vi "Beampointing_sam_edit.vi"() -> ()   [LabVIEW 2020]
uses:
  Ctrs/beam detection.ctl
  GUI_Beampointing_single_TRA/Ctrs/move.ctl
  Shared/GUI_Template/GUI_master/tcp_new_data_event.ctl
  Shared/GUI_Template/GUI_master/tcp new data cluster.ctl
  Ctrs/thresholds.ctl
  Ctrs/Detection all.ctl
  Ctrs/BP configuration.ctl
  General GUIs/Device GUIs/GUI_Cameras/Controls/Crosshair type def.ctl
  <userlib>/_OpenG.lib/array/array.llb/Filter 1D Array with Scalar (String)__ogtk.vi
  <userlib>/_OpenG.lib/array/array.llb/Sort 1D Array (DBL)__ogtk.vi
  <userlib>/_OpenG.lib/array/array.llb/Reorder 1D Array2 (Variant)__ogtk.vi
  <userlib>/_OpenG.lib/file/file.llb/File Exists - Scalar__ogtk.vi
  <userlib>/_OpenG.lib/array/array.llb/Remove Duplicates from 1D Array (String)__ogtk.vi
  <userlib>/_OpenG.lib/file/file.llb/Strip Path Extension - String__ogtk.vi
  <vilib>/Analysis/NI_AALBase.lvlib
  <vilib>/vision/NI_Vision_Development_Module.lvlib
  <vilib>/Utility/file.llb/Write To Spreadsheet File (string).vi
panel:
  in  "pixel calib":dbl
  out "A2y":dbl
  out "A1y":dbl
  out "A2x":dbl
  out "A1x":dbl
  in  "y'":dbl
  in  "x'":dbl
  in  "y":dbl
  in  "x":dbl
  in  "distance to target plane":dbl
  in  "seperation":dbl
  in  "downstream mirror":dbl
  in  "upstream mirror":dbl
  in  "Load Config 2":bool
  out "error out":errorcluster
  in  "active CCDs":i32(listbox)
  out "Prev State":string
  out "tcp data event 2":T1
  out "error out 3":errorcluster
  out "cam means":sgl[](array[numeric])
  in  "save path":path=path "W:/BP_DATA"
  out "millisecond timer value":u32
  out "motor refs 3":refnum<vi>[](array[refnum])
  in  "active man refs":cluster{"Ref X":refnum<vi>, "Ref Y":refnum<vi>}
  in  "#imgs avd so far":dbl
  out "Current State":string
  out "CCDs":string[](array[string])
  in  "GUIdevice 12":string
  in  "GUIdevice 11":string
  in  "GUIdevice 10":string
  in  "GUIdevice 9":string
  out "error out 2":errorcluster
  out "Names":string[](array[string])
  out "Box":T2(array[cluster])
  in  "Tab Cams":T3(tab)=enum."Main"
  in  "Cameras and motors":T4(array[cluster]) {"Motor Alias Y" items=["SHG-angle", "compensation-plate-x", "compensation-plate-y", "Stage [um]", "grating angle", "AttenuatorWavelplate", "Delay", "micrometer", "rail position", "Amp3 North", "djjdjd", "drive grating 2 trans", "speed_translation", "speed_rot_grating2", "speed_rot_grating1", "drive grating 2 rot", "drive grating 1 rot", "jet x", "jet y", "jet z", "ESP2_1_blade", "ESP2_2_target rotation", "home1", "ESP2_3_Scatter ST4 Move", "ESP3_3_mode z position", "com", "ESP3_1_Scatter_Mirror_Z", "ESP3_2", "ESP6_1_scatter ST4 x/hor", "ESP6_2_scatter ST4 y/vert", "ESP6_3_scatter mode z", "VISA", "S1C1 x", "S1C1 y", "S1C1 z", "S1C2 x", "S1C2 y", "S1C2 z", "S1C3 x", "S1C3 y", "S1C3 z", "S1C4 x", "S1C4 y", "S1C4 z", "S2C1 x", "S2C1 y", "S2C1 z", "S2C2 x", "S2C2 y", "S2C2 z", "S2C3 x", "S2C3 y", "S2C3 z", "S2C4 x", "S2C4 y", "S2C4 z", "S3C1 x", "S3C1 y", "S3C1 z", "S3C2 x", "S3C2 y", "S3C2 z", "S3C3 x", "S3C3 y", "S3C3 z", "S3C4 x", "S3C4 y", "S3C4 z", "S4C1 x", "S4C1y", "S4C1 z", "S4C2 x", "S4C2 y", "S4C2 z", "S4C3 x", "S4C3 y", "S4C3 z", "S4C4 x", "S4C4 y", "S4C4 z", "S5C1 x", "S5C1 y", "S5C1 z", "S5C2 x", "S5C2 y", "S5C2 z", "S5C3 x", "S5C3 y", "S5C3 z", "S5C4 x", "S5C4 y", "S5C4 z", "S1C1", "S1C2", "S1C3", "S1C4", "S2C1", "S2C2", "S2C3", "S2C4", "S3C1", "S3C2", "S3C3", "S3C4", "S4C1", "S4C2", "S4C3", "S4C4", "S5C1", "S5C2", "S5C3", "S5C4", "Stepsize 1", "Stepsize 2", "Stepsize 3", "VISA", "S1C1", "S1C2", "S1C3", "S1C4", "S2C1", "S2C2", "S2C3", "S2C4", "S3C1", "S3C2", "S3C3", "S3C4", "S4C1", "S4C2", "S4C3", "S4C4", "S5C1", "S5C2", "S5C3", "S5C4", "kHz EC wedge", "Fiber Mode", "XH2", "ND6", "XH4", "d-scan wedge", "EC wedge", "Lanex", "Gentec", "ModeImager", "Magnet", "ProbeDelay", "x position", "y position", "not working", "LaserDiodeX", "LaserDiodeY", "DelayStage (mm)", "Focus_Beam_2 (mm)", "Hex_x", "Hex_y", "Hex_z", "Hex_u", "Hex_v", "Hex_w", "Mode_Image_pos (mm)", "Jet X", "Jet Y", "Jet Z", "Amp2_out_Y", "Amp3_in_X", "Amp2_out_X", "Amp3_in_Y", "Amp4_in_X", "Amp4_in_Y", "Amp4_in_X", "Gaia2_South_Y", "Gaia3_South_X", "Gaia3_South_Y", "Gaia4_South_X", "Gaia4_South_Y", "Amp2_in_X", "Not Working", "Gaia3_North_X", "Gaia3_North_Y", "Gaia4_North_X", "Gaia4_North_Y", "Expanderin_1_X", "Expanderin_1_Y", "weak current", "Amp4_Out_Y", "Gaia2_North_X", "Gaia2_North_Y", "Amp4_out_X", "Amp2_in_Y", "Gaia2_South_X", "Stretcher_Out_X", "Not_Working", "Stretcher_Out_Y", "JetBladeHeight", "Probe far X", "Probe far Y", "Probe near X", "Probe near Y", "Seed in X", "Seed in Y", "Probe delay X", "Probe delay Y", "Seed Lens Z", "SeedWaveplateRot", "Broken", "SeedPrismBroken", "SeedPrismY", "SeedPrismX", "BCaveDiodeM2Horizontal", "BCaveDiodeM2Vertical", "BCaveDiodeM1Vertical", "BCaveDiodeM1Horizontal", "Grating separation (um)", "Grating1 angle", "Grating2 angle", "Jet_X (mm)", "Jet_Y (mm)", "Jet_Z (mm)", "Prepulse stage", "LegendCompressor (mm)", "devport", "ModeImager", "JetBlade", "ProbeDelay", "1", "TubeIn-x", "TubeIn-y", "CompIn-x", "CompIn-y", "stepSize", "Beamline_In-x", "Beamline_In-y", "Beamline_Out-y", "Beamline_Out-x", "OAPin2-x", "OAPin2-y", "Chassi IP", "BCaveIn-X", "BCaveIn-Y", "OAPIn1-X", "OAPIn1-Y", "DMSurface-X", "DMSurface-Y", "testzaber"]; "Motor Alias X" items=["SHG-angle", "compensation-plate-x", "compensation-plate-y", "Stage [um]", "grating angle", "AttenuatorWavelplate", "Delay", "micrometer", "rail position", "Amp3 North", "djjdjd", "drive grating 2 trans", "speed_translation", "speed_rot_grating2", "speed_rot_grating1", "drive grating 2 rot", "drive grating 1 rot", "jet x", "jet y", "jet z", "ESP2_1_blade", "ESP2_2_target rotation", "home1", "ESP2_3_Scatter ST4 Move", "ESP3_3_mode z position", "com", "ESP3_1_Scatter_Mirror_Z", "ESP3_2", "ESP6_1_scatter ST4 x/hor", "ESP6_2_scatter ST4 y/vert", "ESP6_3_scatter mode z", "VISA", "S1C1 x", "S1C1 y", "S1C1 z", "S1C2 x", "S1C2 y", "S1C2 z", "S1C3 x", "S1C3 y", "S1C3 z", "S1C4 x", "S1C4 y", "S1C4 z", "S2C1 x", "S2C1 y", "S2C1 z", "S2C2 x", "S2C2 y", "S2C2 z", "S2C3 x", "S2C3 y", "S2C3 z", "S2C4 x", "S2C4 y", "S2C4 z", "S3C1 x", "S3C1 y", "S3C1 z", "S3C2 x", "S3C2 y", "S3C2 z", "S3C3 x", "S3C3 y", "S3C3 z", "S3C4 x", "S3C4 y", "S3C4 z", "S4C1 x", "S4C1y", "S4C1 z", "S4C2 x", "S4C2 y", "S4C2 z", "S4C3 x", "S4C3 y", "S4C3 z", "S4C4 x", "S4C4 y", "S4C4 z", "S5C1 x", "S5C1 y", "S5C1 z", "S5C2 x", "S5C2 y", "S5C2 z", "S5C3 x", "S5C3 y", "S5C3 z", "S5C4 x", "S5C4 y", "S5C4 z", "S1C1", "S1C2", "S1C3", "S1C4", "S2C1", "S2C2", "S2C3", "S2C4", "S3C1", "S3C2", "S3C3", "S3C4", "S4C1", "S4C2", "S4C3", "S4C4", "S5C1", "S5C2", "S5C3", "S5C4", "Stepsize 1", "Stepsize 2", "Stepsize 3", "VISA", "S1C1", "S1C2", "S1C3", "S1C4", "S2C1", "S2C2", "S2C3", "S2C4", "S3C1", "S3C2", "S3C3", "S3C4", "S4C1", "S4C2", "S4C3", "S4C4", "S5C1", "S5C2", "S5C3", "S5C4", "kHz EC wedge", "Fiber Mode", "XH2", "ND6", "XH4", "d-scan wedge", "EC wedge", "Lanex", "Gentec", "ModeImager", "Magnet", "ProbeDelay", "x position", "y position", "not working", "LaserDiodeX", "LaserDiodeY", "DelayStage (mm)", "Focus_Beam_2 (mm)", "Hex_x", "Hex_y", "Hex_z", "Hex_u", "Hex_v", "Hex_w", "Mode_Image_pos (mm)", "Jet X", "Jet Y", "Jet Z", "Amp2_out_Y", "Amp3_in_X", "Amp2_out_X", "Amp3_in_Y", "Amp4_in_X", "Amp4_in_Y", "Amp4_in_X", "Gaia2_South_Y", "Gaia3_South_X", "Gaia3_South_Y", "Gaia4_South_X", "Gaia4_South_Y", "Amp2_in_X", "Not Working", "Gaia3_North_X", "Gaia3_North_Y", "Gaia4_North_X", "Gaia4_North_Y", "Expanderin_1_X", "Expanderin_1_Y", "weak current", "Amp4_Out_Y", "Gaia2_North_X", "Gaia2_North_Y", "Amp4_out_X", "Amp2_in_Y", "Gaia2_South_X", "Stretcher_Out_X", "Not_Working", "Stretcher_Out_Y", "JetBladeHeight", "Probe far X", "Probe far Y", "Probe near X", "Probe near Y", "Seed in X", "Seed in Y", "Probe delay X", "Probe delay Y", "Seed Lens Z", "SeedWaveplateRot", "Broken", "SeedPrismBroken", "SeedPrismY", "SeedPrismX", "BCaveDiodeM2Horizontal", "BCaveDiodeM2Vertical", "BCaveDiodeM1Vertical", "BCaveDiodeM1Horizontal", "Grating separation (um)", "Grating1 angle", "Grating2 angle", "Jet_X (mm)", "Jet_Y (mm)", "Jet_Z (mm)", "Prepulse stage", "LegendCompressor (mm)", "devport", "ModeImager", "JetBlade", "ProbeDelay", "1", "TubeIn-x", "TubeIn-y", "CompIn-x", "CompIn-y", "stepSize", "Beamline_In-x", "Beamline_In-y", "Beamline_Out-y", "Beamline_Out-x", "OAPin2-x", "OAPin2-y", "Chassi IP", "BCaveIn-X", "BCaveIn-Y", "OAPIn1-X", "OAPIn1-Y", "DMSurface-X", "DMSurface-Y", "testzaber"]}
  in  "tdms root":path=path "c:/BP_DATAsd"
  out "get pos time":u32
  out "config path":string
  out "tolerances (pix)":dbl[](array[numeric])
  in  "device ini":bool
  in  "Exposure:12":dbl=0.095 min=0.0001 max=1.0 format="%#_6f"
  in  "Triggerdelay::12":dbl=0.003 min=0.0 max=0.09 format="%#_6f"
  in  "Exposure::11":dbl=0.095 min=0.0001 max=1.0 format="%#_6f"
  in  "Triggerdelay::11":dbl=0.003 min=0.0 max=0.09 format="%#_6f"
  in  "Exposure::10":dbl=0.095 min=0.0001 max=1.0 format="%#_6f"
  in  "Triggerdelay::10":dbl=0.003 min=0.0 max=0.09 format="%#_6f"
  in  "Exposure::9":dbl=0.095 min=0.0001 max=1.0 format="%#_6f"
  in  "Triggerdelay::9":dbl=0.003 min=0.0 max=0.09 format="%#_6f"
  in  "Trigger::9":bool
  in  "Trigger::10":bool caption="Trigger:10"
  in  "Trigger::11":bool
  in  "Trigger::12":bool
  in  "Target.Y::9":dbl=45.0 caption="T9y" min=0.0 max=2000.0 format="%#_6f"
  in  "Target.X::9":dbl=47.0 caption="Tx9" min=0.0 max=2000.0 format="%#_6f"
  in  "Target.Y::10":dbl=45.0 caption="T10y" min=0.0 max=2000.0 format="%#_6f"
  in  "Target.X::10":dbl=47.0 caption="T10x" min=0.0 max=2000.0 format="%#_6f"
  in  "Target.Y::11":dbl=45.0 caption="T11y" min=0.0 max=2000.0 format="%#_6f"
  in  "Target.X::11":dbl=47.0 caption="T11x" min=0.0 max=2000.0 format="%#_6f"
  in  "Target.Y::12":dbl=45.0 caption="T12y" min=0.0 max=2000.0 format="%#_6f"
  in  "Target.X::12":dbl=47.0 caption="T12x" min=0.0 max=2000.0 format="%#_6f"
  in  "Exposure::8":dbl=0.095 min=3.8e-05 max=1.0 format="%#_6f"
  in  "Triggerdelay::8":dbl=0.003 min=0.0 max=0.09 format="%#_6f"
  in  "Trigger::8":bool
  in  "Target.Y::8":dbl=45.0 caption="T8y" min=0.0 max=2000.0 format="%#_6f"
  in  "Target.X::8":dbl=47.0 caption="T8x" min=0.0 max=2000.0 format="%#_6f"
  in  "Target.Y::7":dbl=45.0 caption="T7x" min=0.0 max=2000.0 format="%#_6f"
  in  "Target.X::7":dbl=47.0 caption="T7y" min=0.0 max=2000.0 format="%#_6f"
  in  "Target.Y::6":dbl=45.0 caption="T6y" min=0.0 max=2000.0 format="%#_6f"
  in  "Target.X::6":dbl=47.0 caption="T6x" min=0.0 max=2000.0 format="%#_6f"
  in  "Target.Y::5":dbl=45.0 caption="T5y" min=0.0 max=2000.0 format="%#_6f"
  in  "Target.X::5":dbl=47.0 caption="T5x" min=0.0 max=2000.0 format="%#_6f"
  in  "Target.Y::4":dbl=45.0 caption="T4y" min=0.0 max=2000.0 format="%#_6f"
  in  "Target.X::4":dbl=47.0 caption="T4x" min=0.0 max=2000.0 format="%#_6f"
  in  "Target.Y::3":dbl=163.0 caption="T3y" min=0.0 max=2000.0 format="%#_6f"
  in  "Target.X::3":dbl=152.0 caption="T3x" min=0.0 max=2000.0 format="%#_6f"
  in  "Target.Y::2":dbl=74.0 caption="T2y" min=0.0 max=2000.0 format="%#_6f"
  in  "Target.X::2":dbl=75.0 caption="T2x" min=0.0 max=2000.0 format="%#_6f"
  in  "Target.Y::1":dbl=61.0 caption="T1y" min=0.0 max=2000.0 format="%#_6f"
  in  "Target.X::1":dbl=77.0 caption="T1x" min=0.0 max=2000.0 format="%#_6f"
  in  "Exposure::7":dbl=0.095 min=3.8e-05 max=1.0 format="%#_6f"
  in  "Triggerdelay::7":dbl=0.003 min=0.0 max=0.09 format="%#_6f"
  in  "Trigger::7":bool
  in  "Exposure::6":dbl=0.095 min=0.0001 max=1.0 format="%#_6f"
  in  "Triggerdelay::6":dbl=0.003 min=1.0 max=900000.0 format="%#_6f"
  in  "Trigger::6":bool
  in  "Exposure::5":dbl=0.095 min=0.0001 max=1.0 format="%#_6f"
  in  "Triggerdelay::5":dbl=0.003 min=0.0 max=100000.0 format="%#_6f"
  in  "Trigger::5":bool
  in  "Exposure::4":dbl=0.095 min=10.0 max=1000000.0 format="%#_6f"
  in  "Triggerdelay::4":dbl=0.003 min=10.0 max=1000000.0 format="%#_6f"
  in  "Trigger::4":bool
  in  "Exposure::3":dbl=0.095 min=5e-05 max=1.0 format="%#_6f"
  in  "Triggerdelay::3":dbl=0.003 min=10.0 max=500000.0 format="%#_6f"
  in  "Trigger::3":bool
  in  "Exposure::2":dbl=0.095 min=1e-05 max=1.0 format="%#_6f"
  in  "Triggerdelay::2":dbl=0.003 min=10.0 max=100000.0 format="%#_6f"
  in  "Trigger::2":bool
  out "image::1":T5(plugin-control) caption="UC_TubeIn"
  out "image::2":T5(plugin-control) caption="UC_GratingMode"
  out "image::3":T5(plugin-control) caption="UC_DMSurface"
  out "image::4":T5(plugin-control) caption="UC_BCaveIn"
  out "image::5":T5(plugin-control) caption="UC_OAPin1"
  out "image::6":T5(plugin-control) caption="UC_OAPin2"
  out "image::7":T5(plugin-control)
  out "image::8":T5(plugin-control)
  in  "Exposure::1":dbl=0.095 min=50.0 max=500000.0 format="%#_6f"
  in  "Triggerdelay::1":dbl=0.003 min=0.01 max=999000.0 format="%#_6f"
  in  "Trigger::1":bool
  in  "UDP error message":string
  out "required Y":bool[](array[boolean])
  out "required X":bool[](array[boolean])
  out "detected":bool[](array[boolean])
  out "name array":string[](array[string])
  out "image::9":T5(plugin-control)
  out "image::10":T5(plugin-control)
  out "image::11":T5(plugin-control)
  out "image::12":T5(plugin-control)
  out "CCD 1":cluster{timestamp[], dbl[]}[](graph)
  in  "History Size":i32=500
  out "History Index":i32
  in  "Cam# history":i32
  out "Moving X":string
  out "Moving Y":string
  in  "centroidy::4":dbl=45.0 caption="T4y" min=0.0 max=0.0 format="%#_6f"
  in  "centroidx::4":dbl=47.0 caption="T4x" min=0.0 max=0.0 format="%#_6f"
  in  "centroidy::3":dbl=163.0 caption="T3y" min=0.0 max=0.0 format="%#_6f"
  in  "centroidx::3":dbl=152.0 caption="T3x" min=0.0 max=0.0 format="%#_6f"
  in  "centroidy::2":dbl=74.0 caption="T2y" min=0.0 max=0.0 format="%#_6f"
  in  "centroidx::2":dbl=75.0 caption="T2x" min=0.0 max=0.0 format="%#_6f"
  in  "centroidy::1":dbl=61.0 caption="T1y" min=0.0 max=0.0 format="%#_6f"
  in  "centroidx::1":dbl=77.0 caption="T1x" min=0.0 max=0.0 format="%#_6f"
  in  "centroidy::8":dbl=45.0 caption="T8y" min=0.0 max=0.0 format="%#_6f"
  in  "centroidx::8":dbl=47.0 caption="T8x" min=0.0 max=0.0 format="%#_6f"
  in  "centroidy::7":dbl=45.0 caption="T7x" min=0.0 max=0.0 format="%#_6f"
  in  "centroidx::7":dbl=47.0 caption="T7y" min=0.0 max=0.0 format="%#_6f"
  in  "centroidy::6":dbl=45.0 caption="T6y" min=0.0 max=0.0 format="%#_6f"
  in  "centroidx::6":dbl=47.0 caption="T6x" min=0.0 max=0.0 format="%#_6f"
  in  "centroidy::5":dbl=45.0 caption="T5y" min=0.0 max=0.0 format="%#_6f"
  in  "centroidx::5":dbl=47.0 caption="T5x" min=0.0 max=0.0 format="%#_6f"
  in  "centroidy::12":dbl=45.0 caption="T12y" min=0.0 max=2000.0 format="%#_6f"
  in  "centroidx::12":dbl=47.0 caption="T12x" min=0.0 max=2000.0 format="%#_6f"
  in  "centroidy::11":dbl=45.0 caption="T11y" min=0.0 max=2000.0 format="%#_6f"
  in  "centroidx::11":dbl=47.0 caption="T11x" min=0.0 max=2000.0 format="%#_6f"
  in  "centroidy::10":dbl=45.0 caption="T10y" min=0.0 max=2000.0 format="%#_6f"
  in  "centroidx::10":dbl=47.0 caption="T10x" min=0.0 max=2000.0 format="%#_6f"
  in  "centroidy::9":dbl=45.0 caption="T9y" min=0.0 max=2000.0 format="%#_6f"
  in  "centroidx::9":dbl=47.0 caption="Tx9" min=0.0 max=2000.0 format="%#_6f"
  out "active ccd particles":T6(array[cluster])
  in  "Speedmode":dbl=5.0 min=1.0 max=20.0
  in  "Feedback Global":bool
  in  "GUIdevice 8":string
  in  "Tab Control":T7(tab)
  in  "alarms":bool
  in  "new tdms":bool
  in  "Save Stats":bool
  in  "Save Config":bool
  in  "Load Config":bool
  in  "update speed [ms]":i32=2000 min=1000 max=10000
  in  "img to avg":i32=15 min=3 max=200
  in  "Reset History":bool
  in  "autodetect":bool
  in  "Detection Rate":dbl=0.9 min=0.001 max=1.0
  in  "Center":bool
  in  "Align":bool
  in  "average centroid":bool
  in  "clear error":bool
  in  "beam detection para":T8={"Filter"=1, "Filter Para"={"X Size"=5, "Y Size"=5, "% Tolerance"=1}, "detection method"=4, "Particle filtering"=[{"Measurement Parameter"=35, "Range Lower Value"=0.0, "Range Upper Value"=500.0, "Range"=FALSE, "Measurement Type"=FALSE}], "Remove small Objects"=TRUE, "Restrict to round Objects"=FALSE, "Use Cam COM"=FALSE} {"Particle filtering"."Measurement Parameter" items=["Center of Mass X", "Center of Mass Y", "First Pixel X", "First Pixel Y", "Bounding Rect Left", "Bounding Rect Top", "Bounding Rect Right", "Bounding Rect Bottom", "Max Feret Diameter Start X", "Max Feret Diameter Start Y", "Max Feret Diameter End X", "Max Feret Diameter End Y", "Max Horiz. Segment Length Left", "Max Horiz. Segment Length Right", "Max Horiz. Segment Length Row", "-", "Bounding Rect Width", "Bounding Rect Height", "Bounding Rect Diagonal", "Perimeter", "Convex Hull Perimeter", "Holes' Perimeter", "Max Feret Diameter", "Equivalent Ellipse Major Axis", "Equivalent Ellipse Minor Axis", "Equivalent Ellipse Minor Axis (Feret)", "Equivalent Rect Long Side", "Equivalent Rect Short Side", "Equivalent Rect Diagonal", "Equivalent Rect Short Side (Feret)", "Average Horiz. Segment Length", "Average Vert. Segment Length", "Hydraulic Radius", "Waddel Disk Diameter", "-", "Area", "Holes' Area", "Particle & Holes' Area", "Convex Hull Area", "Image Area", "-", "Number of Holes", "Number of Horiz. Segments", "Number of Vert. Segments", "-", "Orientation", "Max Feret Diameter Orientation", "-", "% Area/Image Area", "% Area/(Particle & Holes' Area)", "Ratio of Equivalent Ellipse Axes", "Ratio of Equivalent Rect Sides", "-", "Elongation Factor", "Compactness Factor", "Heywood Circularity Factor", "Type Factor", "-", "Sum X", "Sum Y", "Sum XX", "Sum XY", "Sum YY", "Sum XXX", "Sum XXY", "Sum XYY", "Sum YYY", "-", "Moment of Inertia XX", "Moment of Inertia XY", "Moment of Inertia YY", "Moment of Inertia XXX", "Moment of Inertia XXY", "Moment of Inertia XYY", "Moment of Inertia YYY", "Norm. Moment of Inertia XX", "Norm. Moment of Inertia XY", "Norm. Moment of Inertia YY", "Norm. Moment of Inertia XXX", "Norm. Moment of Inertia XXY", "Norm. Moment of Inertia XYY", "Norm. Moment of Inertia YYY", "Hu Moment 1", "Hu Moment 2", "Hu Moment 3", "Hu Moment 4", "Hu Moment 5", "Hu Moment 6", "Hu Moment 7"]; "Particle filtering"."Range Lower Value" format="%.2f"; "Particle filtering"."Range Upper Value" format="%.2f"; "detection method" items=["clustering", "entropy", "metric", "moments", "inter-class variance"]; "Filter" items=["No Filter", "Median Filter", "Low Pass Filter"]}
  out "Active CCD":string
  in  "thresholds":T10
  in  "move config":T11={"Tolerance [%]"=0.1, "Stepsize"=0.0001, "Invert Direction X"=FALSE, "Invert Direction Y"=TRUE, "enable feedback"=FALSE, "Set Centriod Target"=FALSE, "xCal"=0.0001, "xCal neg"=0.0001, "yCal"=0.0001, "yCal neg"=0.0001}
  in  "Position 2":dbl=0.001 caption="Stepsize" min=0.0 max=999999.0 format="%_6f"
  in  "Position 1":dbl=0.001 caption="Stepsize" min=0.0 max=999999.0 format="%_6f"
  in  "Right":bool caption="RelativeMove.Axis 1.CCW::1"
  in  "Left":bool caption="RelativeMove.Axis 1.CW::1"
  in  "Down":bool caption="RelativeMove.Axis. 2.CCW::1"
  in  "Up":bool caption="RelativeMove.Axis 2.CW::1"
  in  "StepSize":dbl=0.01 caption="Stepsize" min=0.0 max=1.0 step=0.001 format="%#_6p"
  in  "Time":timestamp[][](array[timestamp])
  in  "Offset X":dbl[][](array[numeric])
  in  "Mean Centroid X":dbl[][](array[numeric])
  in  "GUIdevice 7":string
  in  "GUIdevice 6":string
  in  "GUIdevice 5":string
  in  "GUIdevice 4":string
  in  "GUIdevice 3":string="TargetCam10Hz_Diode"
  in  "GUIdevice 2":string="StagingM1Far"
  in  "insert tag":bool=TRUE
  in  "stop":bool
  in  "GUIdevice 1":string="StagingM1Near"
  out "error IO 2":errorcluster
  # "Coupled mirror move (in progress: SAM)"
  # "Motor axes must have aliases"
  # "Save config after changing cams/motors"
  # "max"
  # "When running for the first time\nCancel the load configuration\nSet the Camera and motors in the config tab\nSave the configuration\nLoad the configuration\nConfigure the detection and feedback for each camera\nSave the configuration\n\nTips\nIn detection, you can exclude or include particles. Typically, include based on the area of the particle.\nYou can either use the particle centroid, or the center of mass calculated in the camera\nFor the case of camera COM, it will only use it if it is in the bounding box of the detected particle.\nA calibration is critical for good performance. Use MC to perform a motor scan and perform a linear fit of COM vs motor position in x and y. Put the gradients into xCal and yCal.\nStep size in move config no longer used.\nFor motors (like LTAs), set the backlash and set it to default in MC. Backlash amount is retrieved from a positive and negative motor scan, and reading the position distance between the lines of the graph of COM vs motor position.\nUnder system tab, update speed must be > than slowest camera update. Otherwise program will find the slow cam/s not having a new image, and it will perform a new configuration."
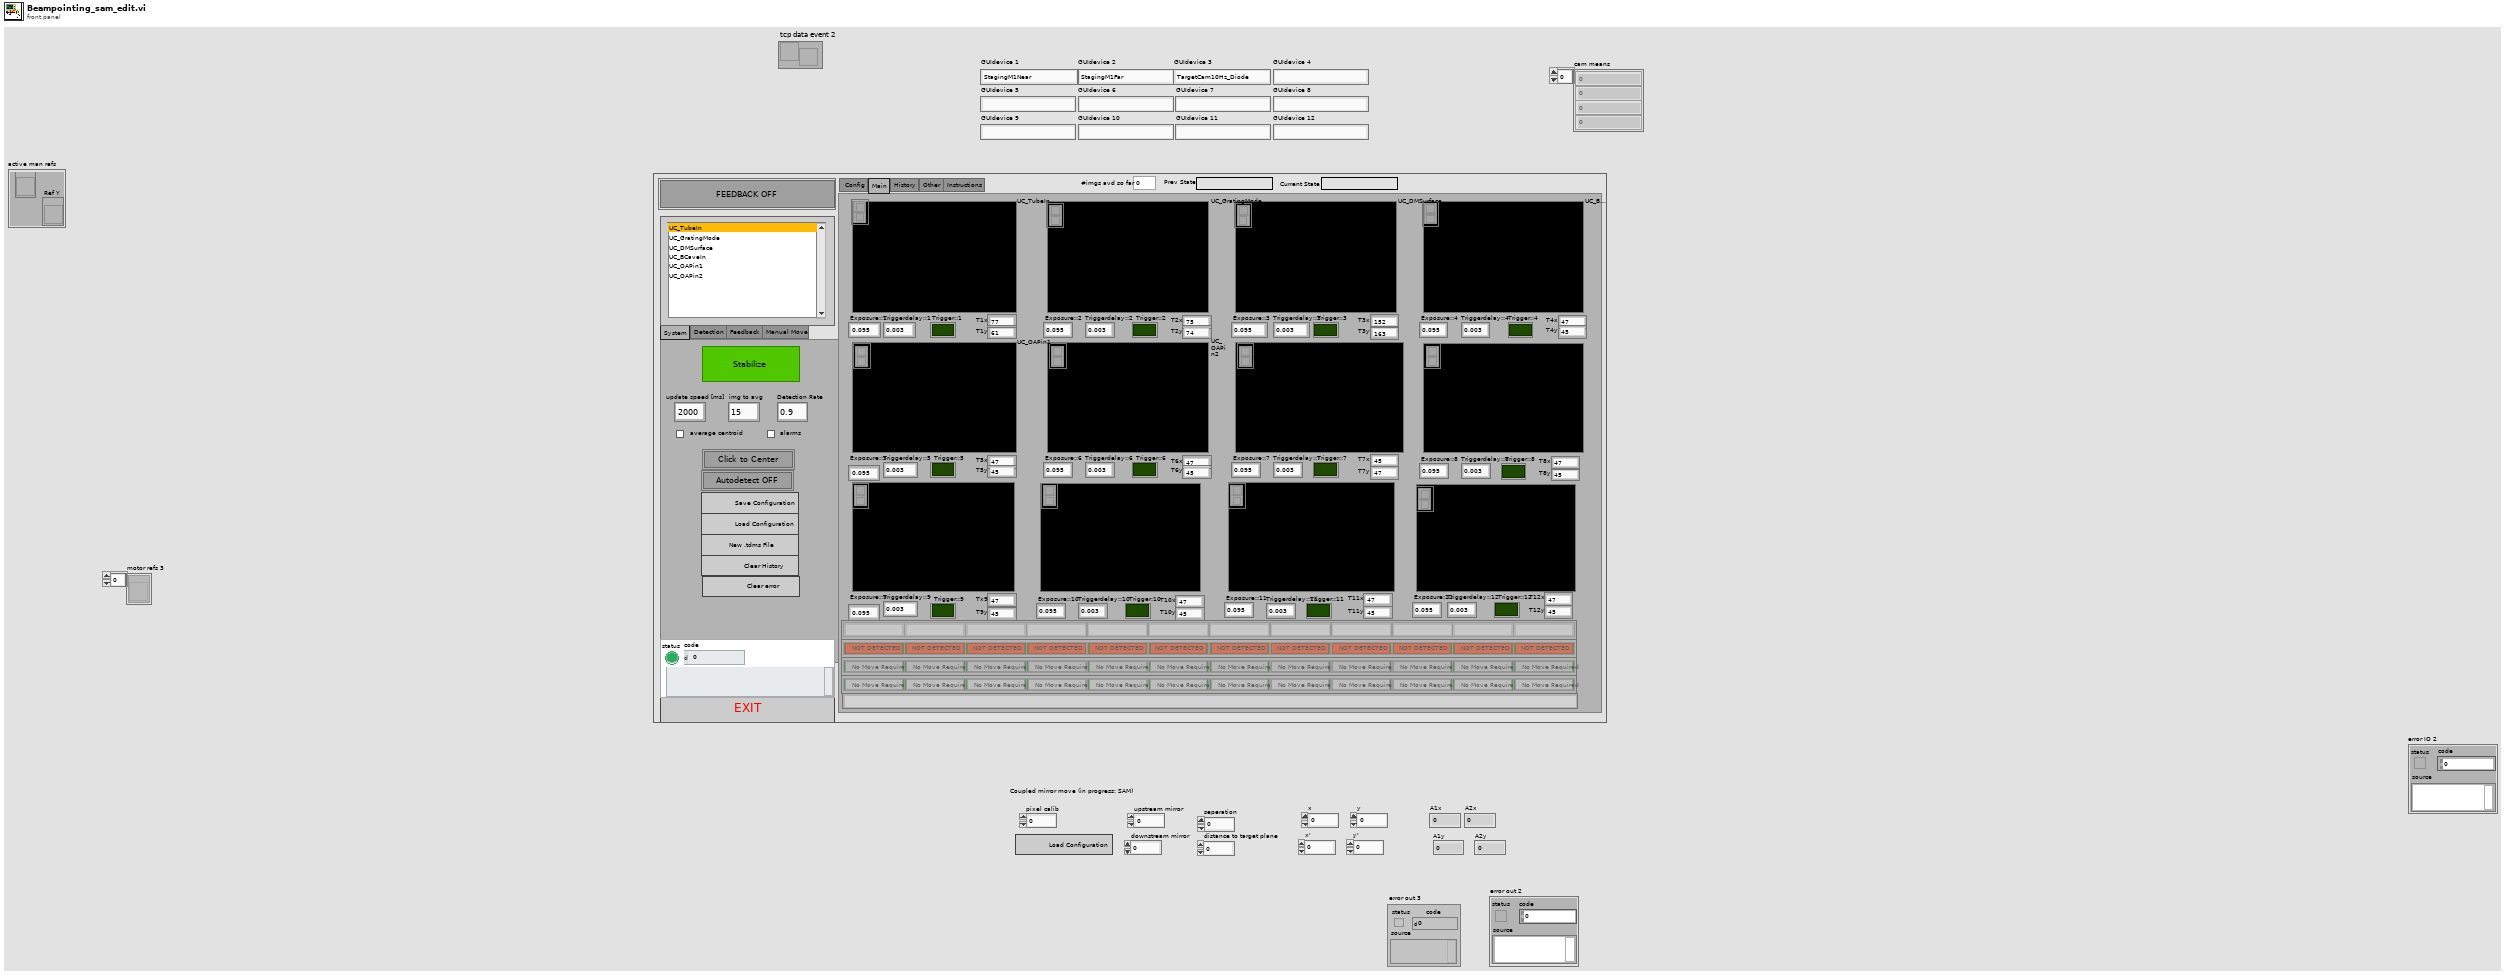
[diagram p1: front panel]
types:
  T1 = typedef "tcp_new_data_event.ctl" = refnum<user-event>
  T2 = cluster{"Left":dbl, "Top":dbl, "Right":dbl, "Bottom":dbl}[]
  T3 = enum32{"Config ", "Main", "History", "Other", "Instructions"}
  T4 = cluster{"Camera":string, "Motor Alias X":u16, "Motor Alias Y":u16}[]
  T5 = typedef "IMAQ Image.ctl" = refnum<image>
  T6 = cluster{"Area":dbl, "Number of Holes":dbl, "Bounding Rect":cluster{"Left":dbl, "Top":dbl, "Right":dbl, "Bottom":dbl}, "Center of Mass":cluster{"X":dbl, "Y":dbl}, "Orientation":dbl, "Dimensions":cluster{"Width":dbl, "Height":dbl}}[]
  T7 = enum32{"System", "Detection", "Feedback", "Manual Move"}
  T8 = typedef "beam detection.ctl" = cluster{"Filter":u16, "Filter Para":cluster{"X Size":i32, "Y Size":i32, "% Tolerance":i32}, "detection method":i32, "Particle filtering":cluster{"Measurement Parameter":T9, "Range Lower Value":dbl, "Range Upper Value":dbl, "Range":bool, "Measurement Type":bool}[], "Remove small Objects":bool, "Restrict to round Objects":bool, "Use Cam COM":bool}
  T9 = typedef "Particle Parameters" = i32
  T10 = typedef "thresholds.ctl" = cluster{"Lower value":sgl, "Upper value":sgl}
  T11 = typedef "move.ctl" = cluster{"Tolerance [%]":dbl, "Stepsize":dbl, "Invert Direction X":bool, "Invert Direction Y":bool, "enable feedback":bool, "Set Centriod Target":bool, "xCal":dbl, "xCal neg":dbl, "yCal":dbl, "yCal neg":dbl}
  T12 = cluster{"Target.X::1":refnum<vi>, "Target.Y::1":refnum<vi>}
  T13 = cluster{"Target.X::2":refnum<vi>, "Target.Y::2":refnum<vi>}
  T14 = cluster{"Target.X::3":refnum<vi>, "Target.Y::3":refnum<vi>}
  T15 = cluster{"Target.X::4":refnum<vi>, "Target.Y::4":refnum<vi>}
  T16 = cluster{"Target.X::5":refnum<vi>, "Target.Y::5":refnum<vi>}
  T17 = cluster{"Target.X::6":refnum<vi>, "Target.Y::6":refnum<vi>}
  T18 = cluster{"Target.X::7":refnum<vi>, "Target.Y::7":refnum<vi>}
  T19 = cluster{"Target.X::8":refnum<vi>, "Target.Y::8":refnum<vi>}
  T20 = cluster{"Target.X::12":refnum<vi>, "Target.Y::12":refnum<vi>}
  T21 = cluster{"Target.X::9":refnum<vi>, "Target.Y::9":refnum<vi>}
  T22 = cluster{"Target.X::10":refnum<vi>, "Target.Y::10":refnum<vi>}
  T23 = cluster{"Target.X::11":refnum<vi>, "Target.Y::11":refnum<vi>}
  T24 = cluster{"Target.X::12":refnum<vi>, "Target.Y::12":refnum<vi>}[]
  T25 = enum32{"invalid app kind", "Development System", "Run Time System", "Student Edition", "Embedded LabVIEW", "Evaluation", "Custom"}
  T26 = enum32{"Invalid", "Standard", "Closed", "Hidden", "Minimized", "Maximized"}
  T27 = typedef "BP configuration.ctl" = cluster{"Camera names":string[], "Motor aliases x":string[], "Motor aliases y":string[], "detection para":T8[], "thresholds":cluster{"Lower value":sgl, "Upper value":sgl}[], "move properties":T11[], "tdms root":path}
  T28 = typedef "tcp new data cluster.ctl" = cluster{"EventEnum":enum16{"new data", "connection status update"}, "Device name":string}
  T29 = enum16{"open", "replace", "create", "open or create", "replace or create", "replace or create with confirmation"}
  T30 = enum8{"Enabled", "Disabled", "Disabled and Grayed Out"}
  T31 = enum16{"open", "open or create", "create or replace", "create", "open (read-only)"}
  T32 = typedef "Detection all.ctl" = cluster{"detection para":T8[], "thresholds":cluster{"Lower value":sgl, "Upper value":sgl}[], "Centroid X":dbl[][], "Centroid Y":dbl[][], "Size":dbl[][], "Centroid refs":cluster{"centroidx::12":refnum<vi>, "centroidy::12":refnum<vi>}[], "img to avg":i32}
  T33 = cluster{"detection para":T8[], "thresholds":cluster{"Lower value":sgl, "Upper value":sgl}[], "Centroid X":dbl[][], "Centroid Y":dbl[][], "Size":dbl[][], "Centroid refs":cluster{"centroidx::12":refnum<vi>, "centroidy::12":refnum<vi>}[], "img to avg":i32}
  T34 = cluster{"Area":dbl, "Number of Holes":dbl, "Bounding Rect":cluster{"Left":dbl, "Top":dbl, "Right":dbl, "Bottom":dbl}, "Center of Mass":cluster{"X":dbl, "Y":dbl}, "Orientation":dbl, "Dimensions":cluster{"Width":dbl, "Height":dbl}}[][]
  T35 = cluster{"Core":cluster{"Current VI Reference":refnum<vi>, "Close Panel on Exit?":bool}, "Detection":T32, "Mean Centroid X":dbl[][], "Mean Centroid Y":dbl[][], "Offset X":dbl[][], "Offset Y":dbl[][], "Offset X stats ":dbl[][], "Offset Y stats ":dbl[][], "Mean Size":dbl[][], "Time":timestamp[][], "move properties":T11[], "active axis refs 2":cluster{"Ref X":refnum<vi>, "Ref Y":refnum<vi>}[], "active ccd":i32, "Feedback global":bool, "Motor X":dbl[][], "Motor Y":dbl[][], "active cams":string[], "tdms ref":refnum<k34>, "active man refs":cluster{"Ref X":refnum<vi>, "Ref Y":refnum<vi>}, "detected":bool[], "speedmode X":bool[], "speedmode Y":bool[], "steps speed X":dbl[], "steps speed Y":dbl[], "Supergui":cluster{"STOP queue":refnum<queue>, "SuperGUI ref":refnum<vi>}, "dev var alias arrays":cluster{"dev variable alias":string[][], "dev variable alias Motors X":string[][], "dev variable alias Motors Y":string[][]}, "Motor positions":cluster{"Positions x":dbl[], "Positions y":dbl[]}, "Config loaded":bool}
  T36 = cluster{"Positions x":dbl[], "Positions y":dbl[]}
  T37 = cluster{"dev variable alias":string[][], "dev variable alias Motors X":string[][], "dev variable alias Motors Y":string[][]}
  T38 = cluster{"Ref X":refnum<vi>, "Ref Y":refnum<vi>}[]
  T39 = cluster{"STOP queue":refnum<queue>, "SuperGUI ref":refnum<vi>}
  T40 = cluster{"Current VI Reference":refnum<vi>, "Close Panel on Exit?":bool}
  T41 = cluster{"centroidx::1":refnum<vi>, "centroidy::1":refnum<vi>}
  T42 = cluster{"centroidx::2":refnum<vi>, "centroidy::2":refnum<vi>}
  T43 = cluster{"centroidx::3":refnum<vi>, "centroidy::3":refnum<vi>}
  T44 = cluster{"centroidx::4":refnum<vi>, "centroidy::4":refnum<vi>}
  T45 = cluster{"centroidx::5":refnum<vi>, "centroidy::5":refnum<vi>}
  T46 = cluster{"centroidx::6":refnum<vi>, "centroidy::6":refnum<vi>}
  T47 = cluster{"centroidx::7":refnum<vi>, "centroidy::7":refnum<vi>}
  T48 = cluster{"centroidx::8":refnum<vi>, "centroidy::8":refnum<vi>}
  T49 = cluster{"centroidx::12":refnum<vi>, "centroidy::12":refnum<vi>}
  T50 = cluster{"centroidx::9":refnum<vi>, "centroidy::9":refnum<vi>}
  T51 = cluster{"centroidx::10":refnum<vi>, "centroidy::10":refnum<vi>}
  T52 = cluster{"centroidx::11":refnum<vi>, "centroidy::11":refnum<vi>}
  T53 = cluster{"centroidx::12":refnum<vi>, "centroidy::12":refnum<vi>}[]
  T54 = cluster{"Camera":string, "Motor Alias X":u16, "Motor Alias Y":u16}
  T55 = typedef "Image Type" = u32
  T56 = cluster{"appended array":timestamp[], "appended array":dbl[]}
  T57 = cluster{"appended array":timestamp[], "appended array":dbl[]}[]
  T58 = typedef "Crosshair type def.ctl" = cluster{"Draw":bool, "Target":cluster{"x":dbl, "y":dbl}, "Size":cluster{"x":dbl, "y":dbl}, "Angle":dbl, "Color":u32, "Thickness":u8, "CrosshairLabel":string}
  T59 = cluster{"Left":i32, "Top":i32, "Right":i32, "Bottom":i32}
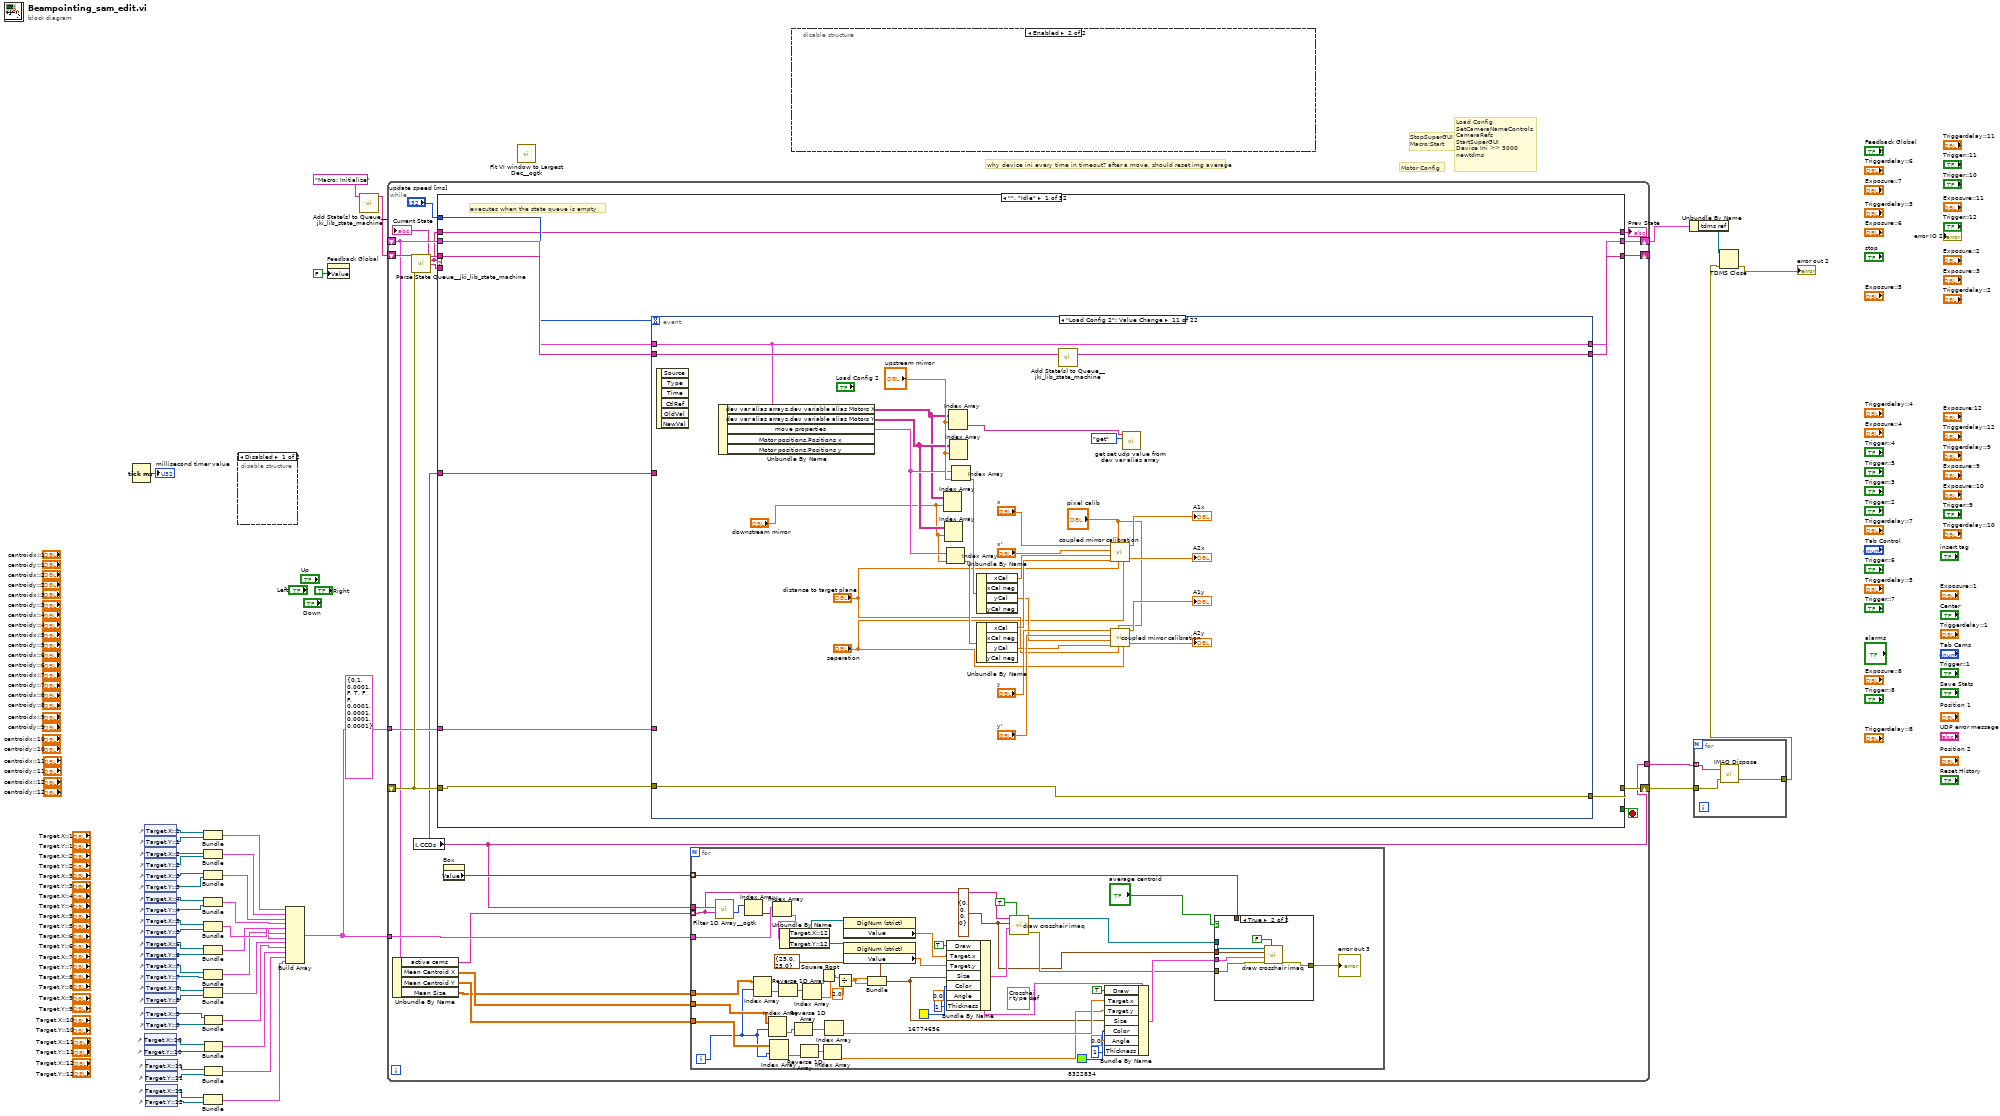
[diagram p0: block diagram]
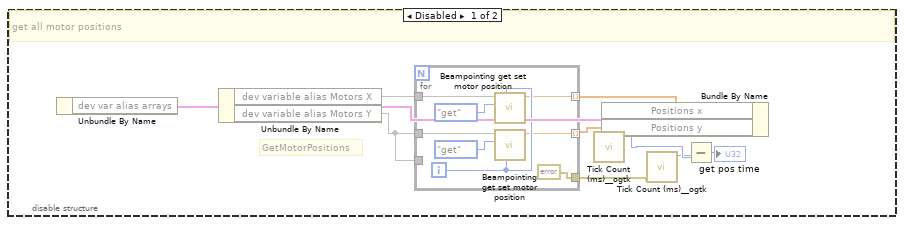
[diagram p2: hidden frame]
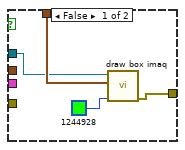
[diagram p4: hidden frame]
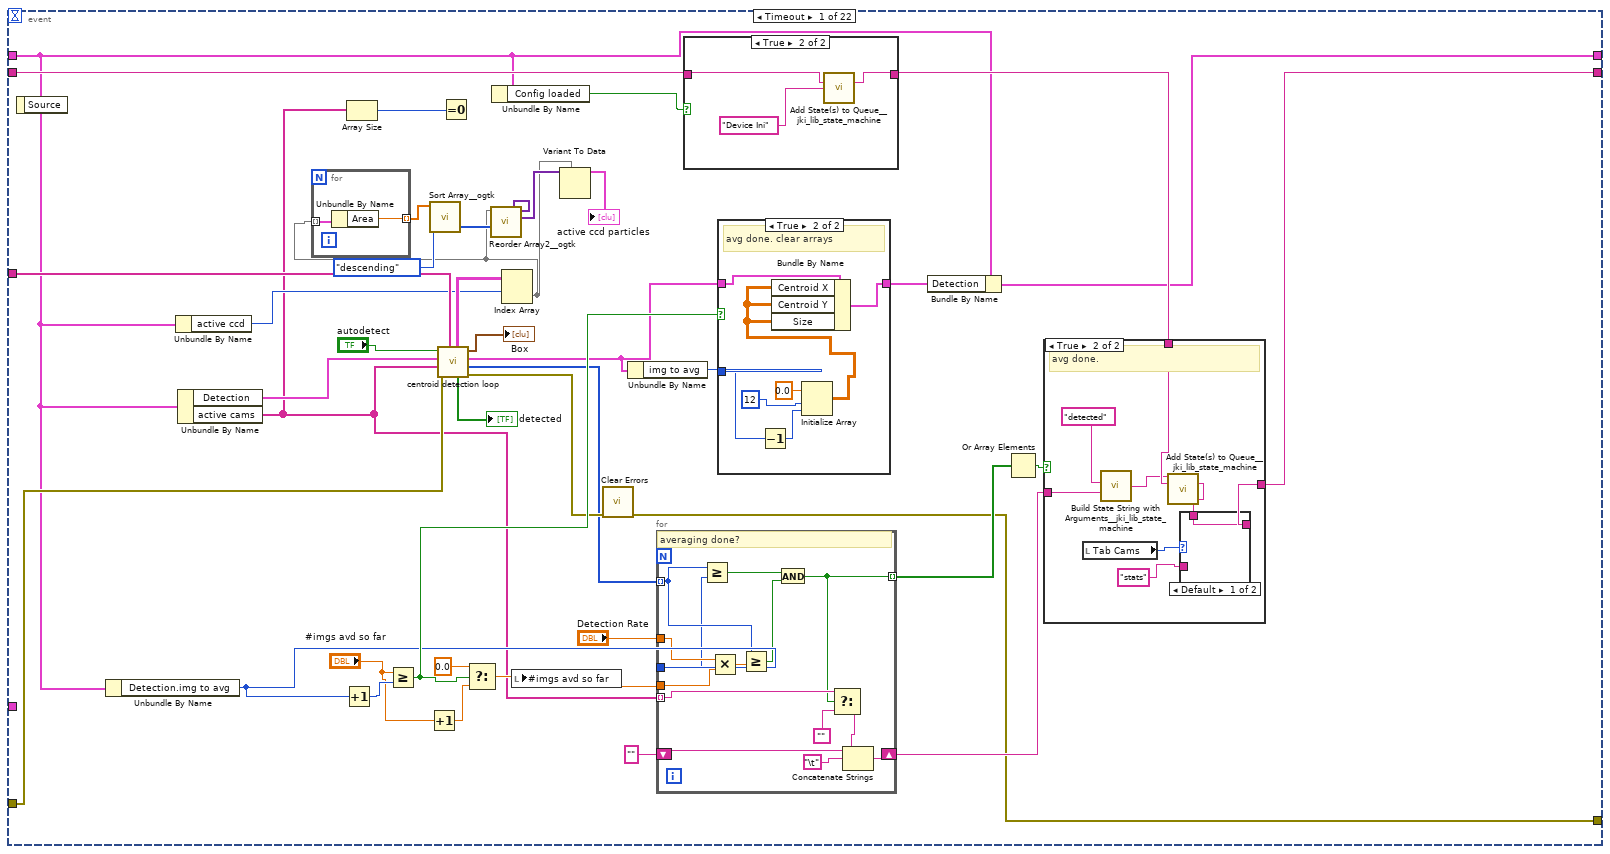
[diagram p5: hidden frame]
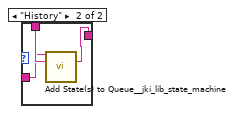
[diagram p9: hidden frame]
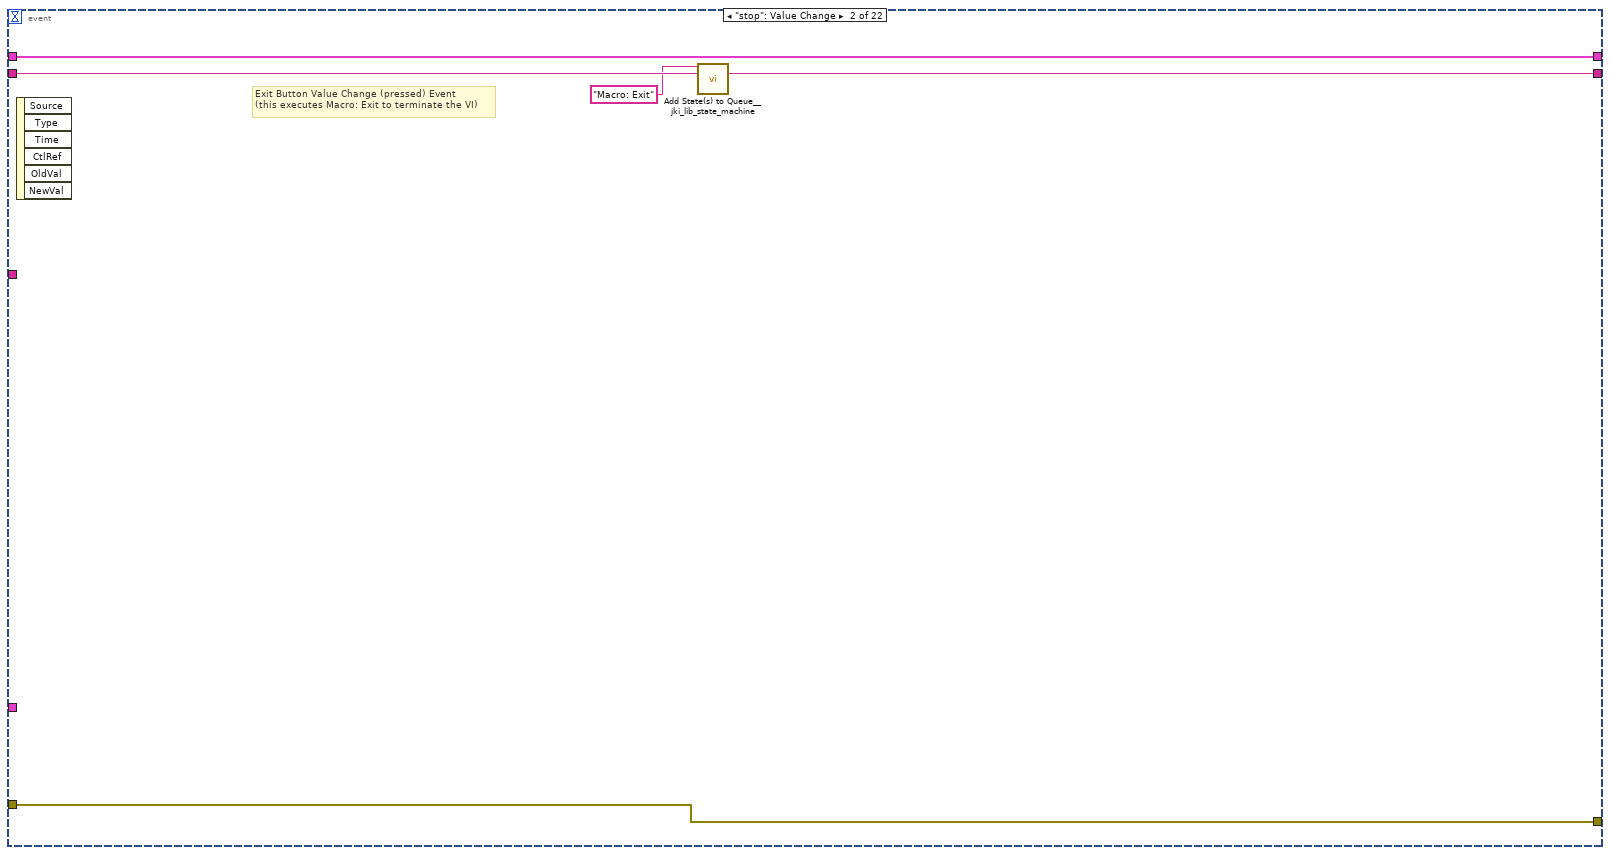
[diagram p10: hidden frame]
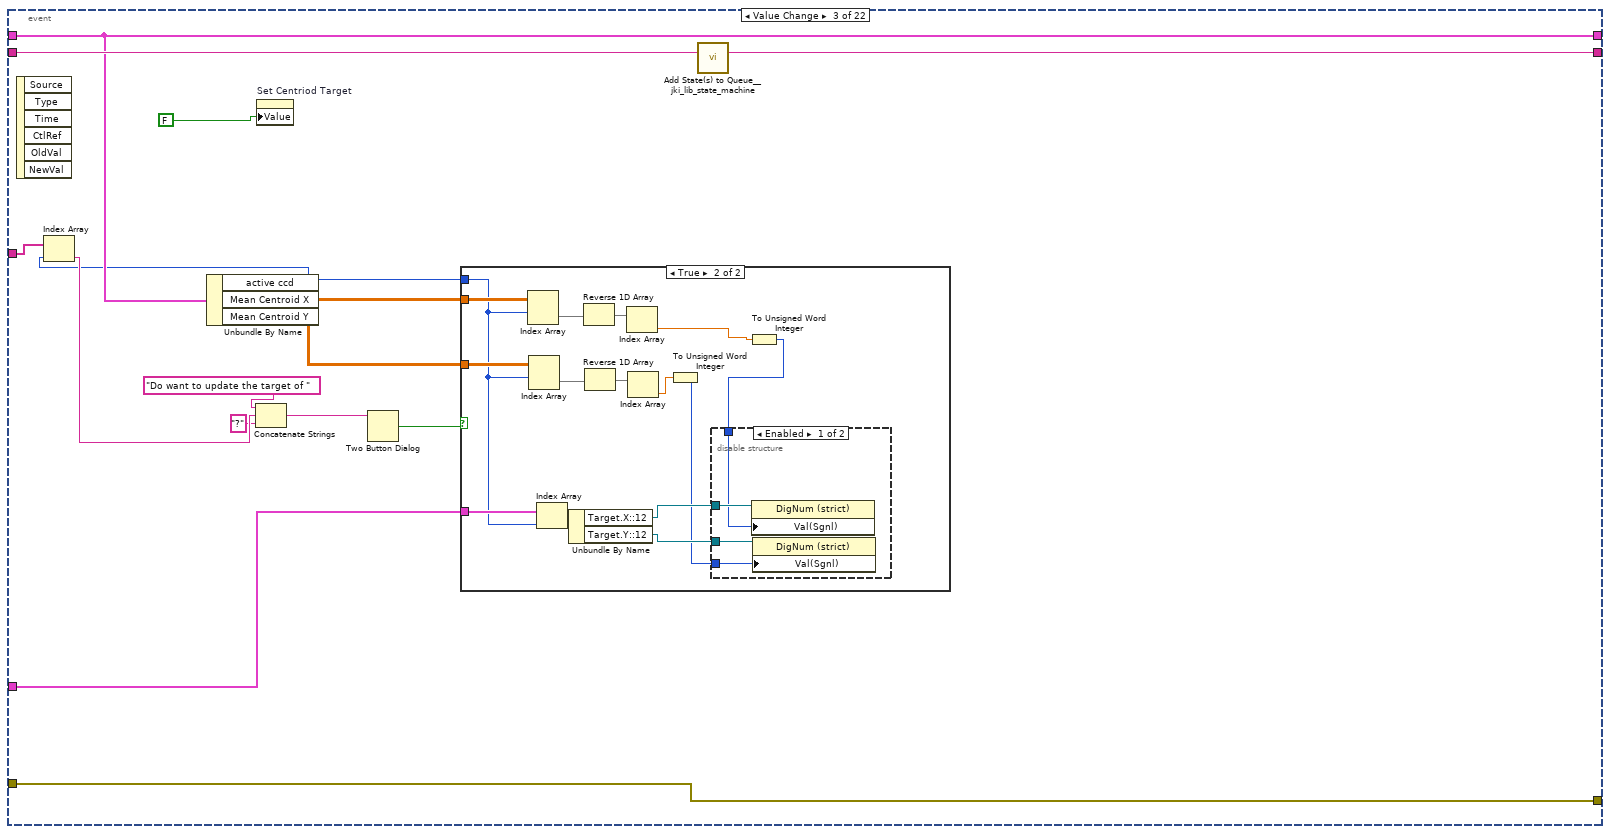
[diagram p11: hidden frame]
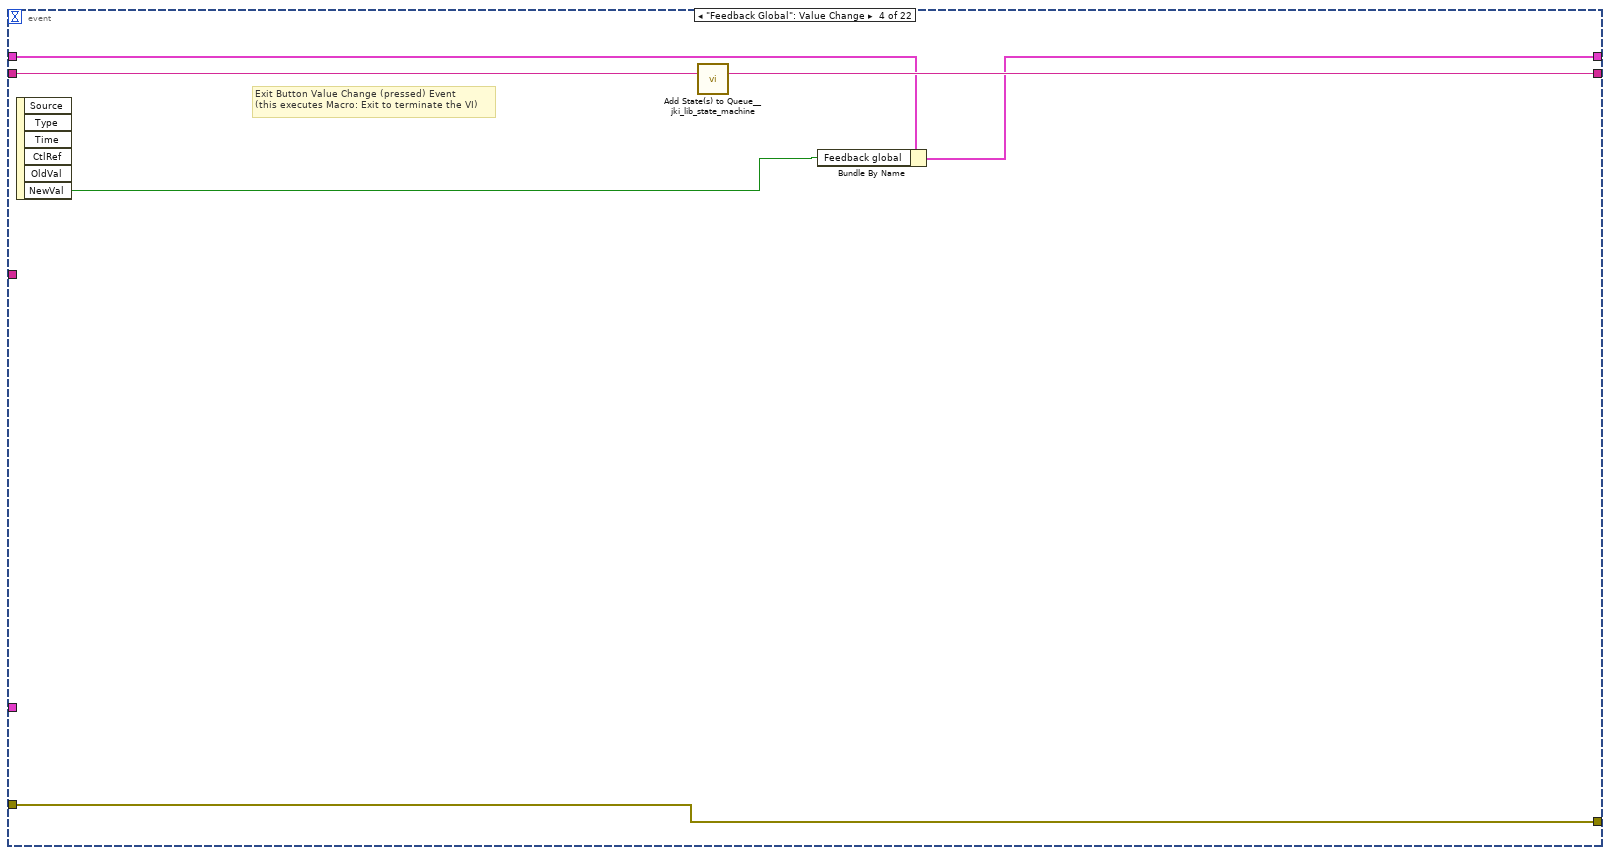
[diagram p14: hidden frame]
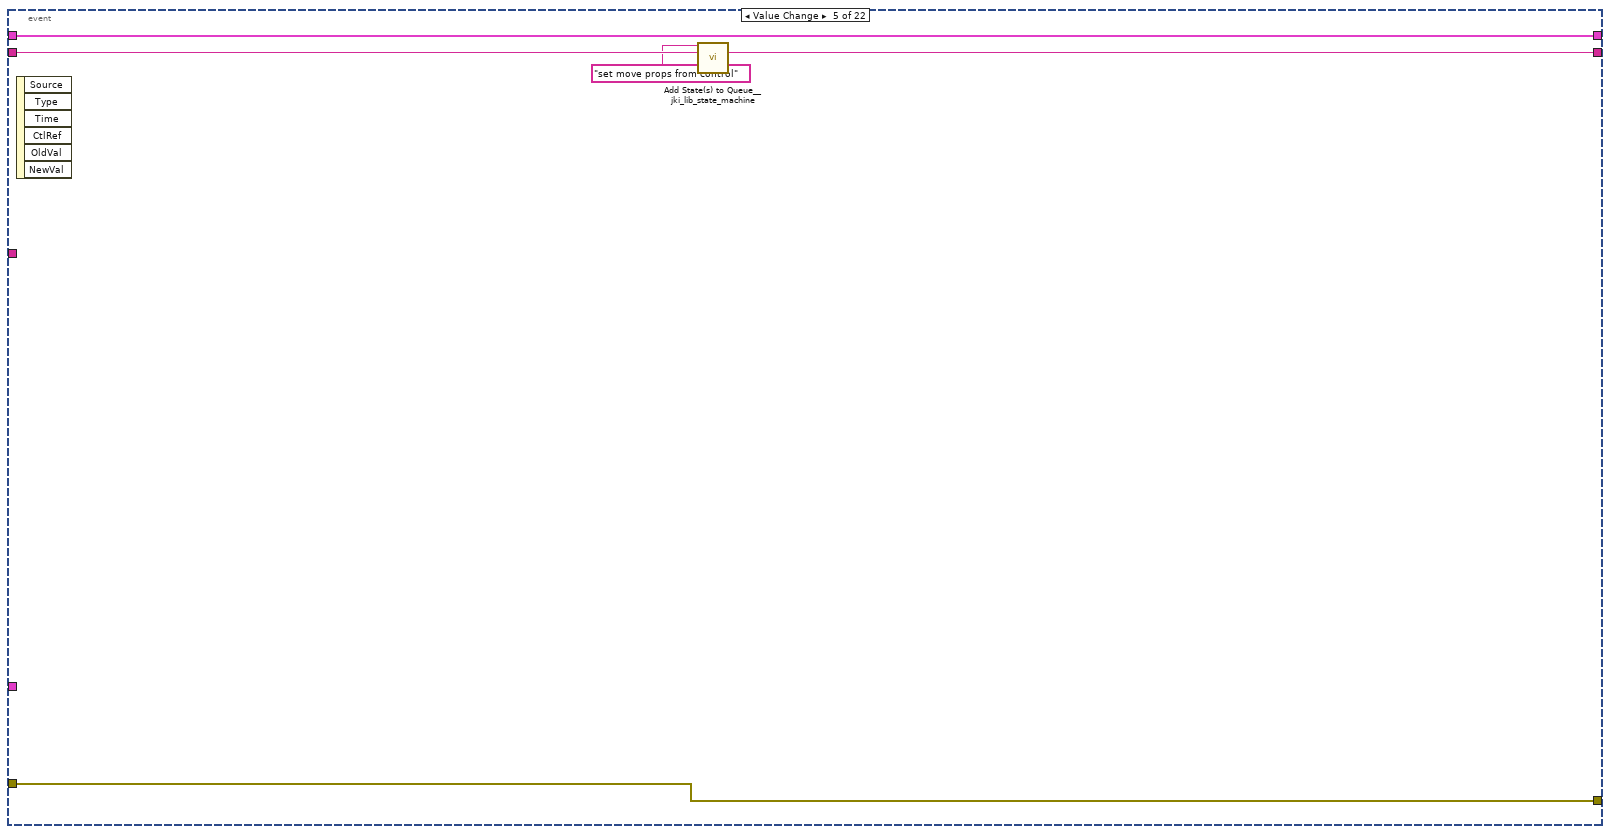
[diagram p15: hidden frame]
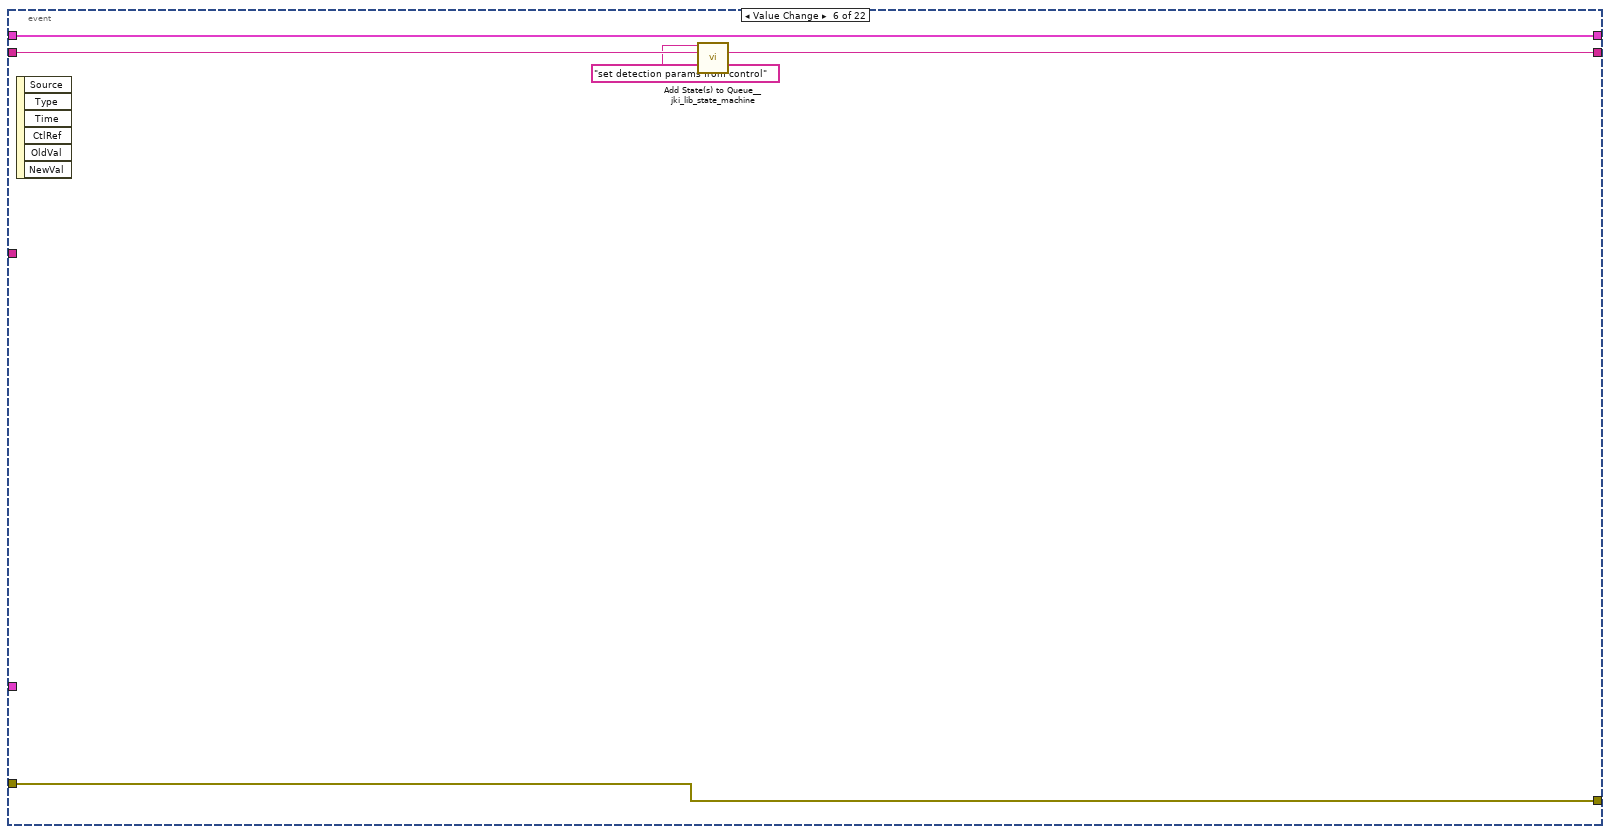
[diagram p16: hidden frame]
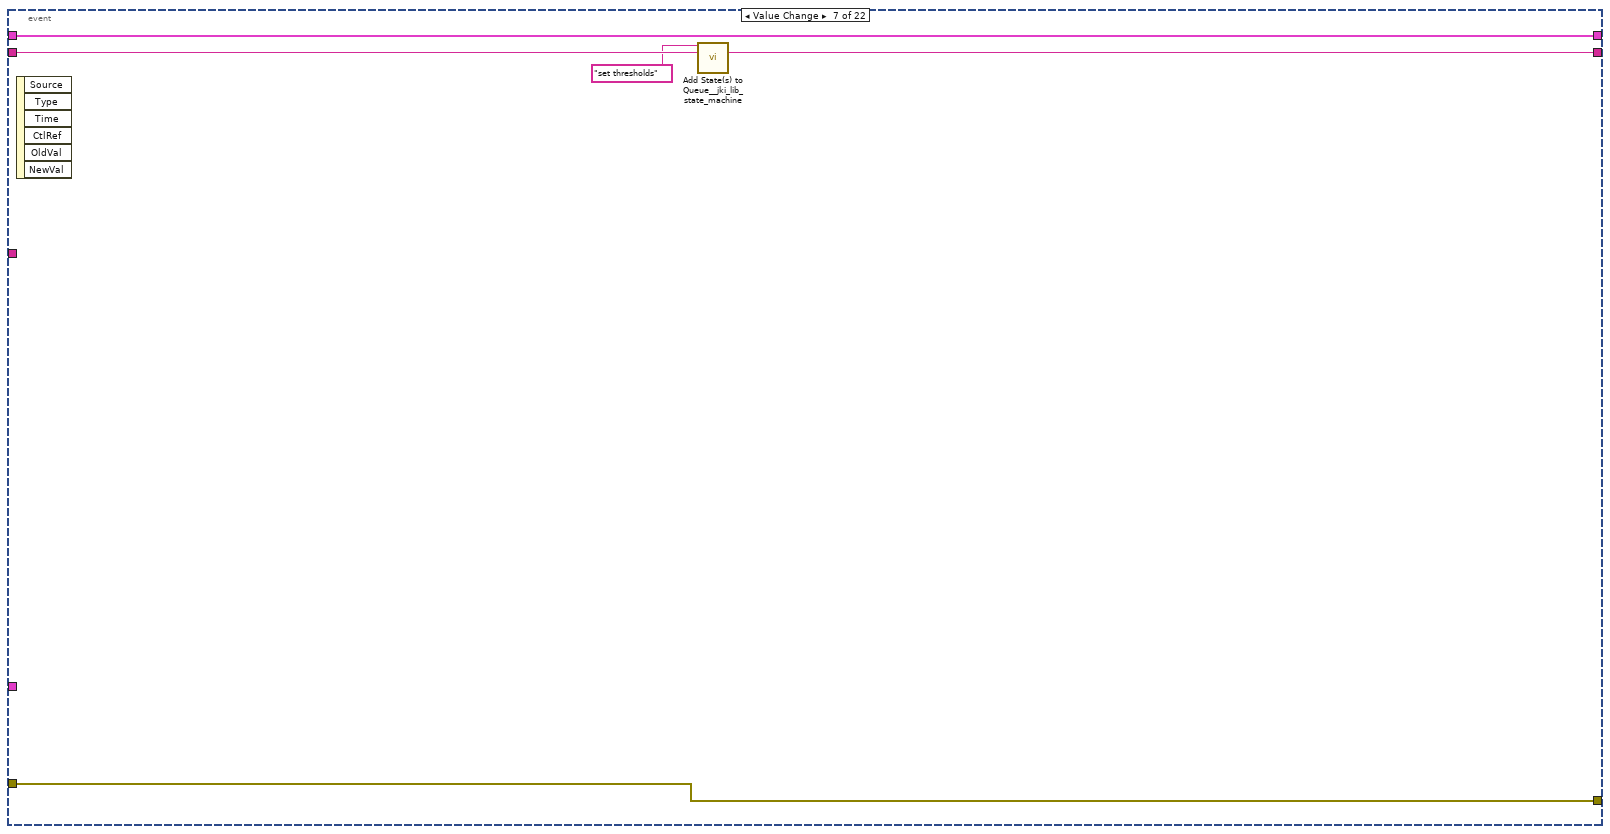
[diagram p17: hidden frame]
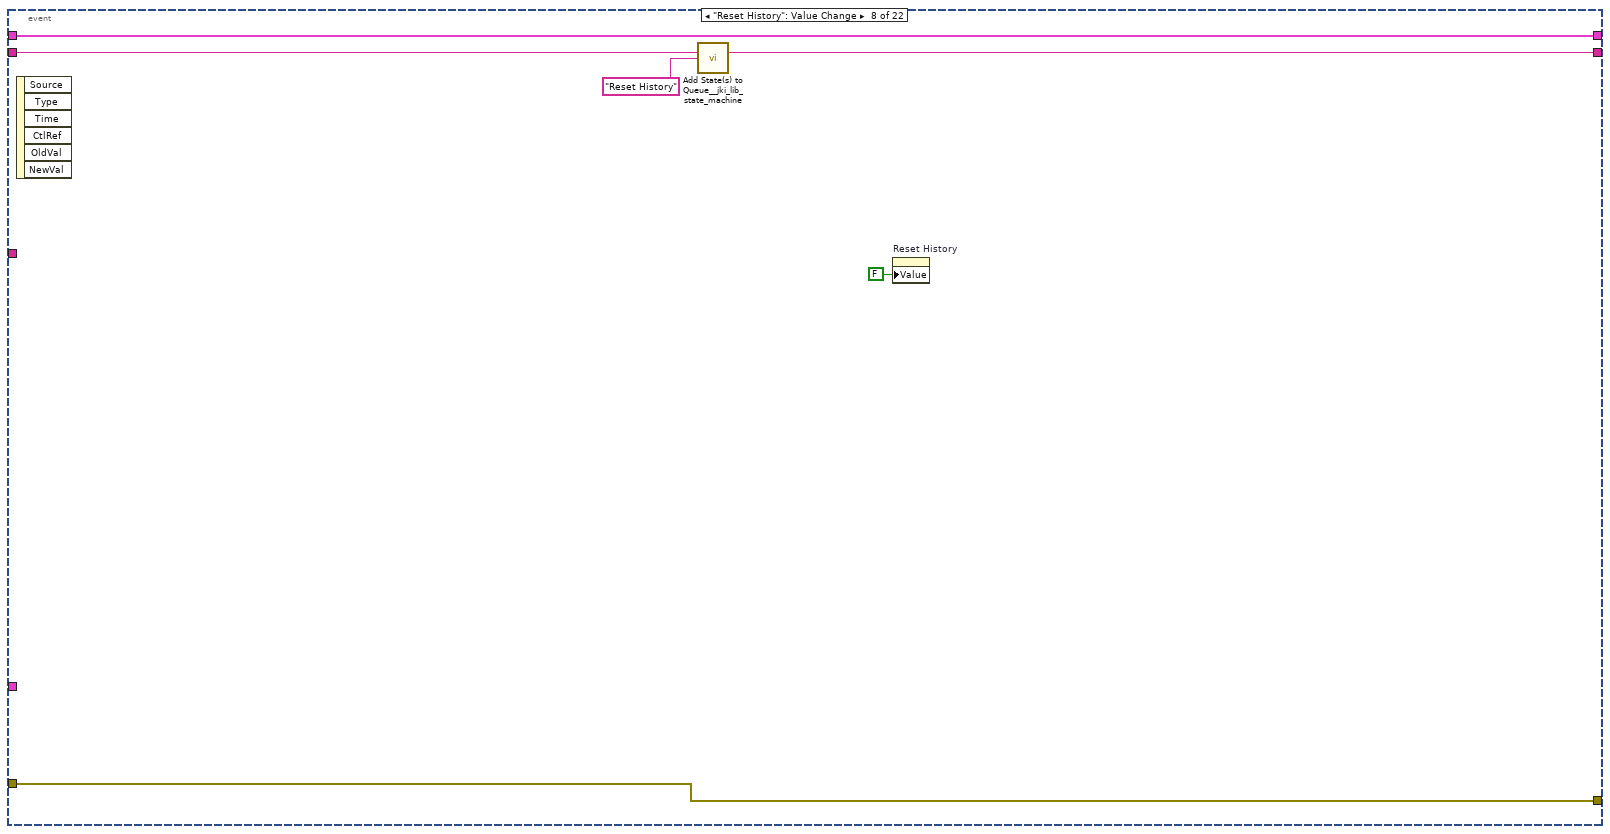
[diagram p18: hidden frame]
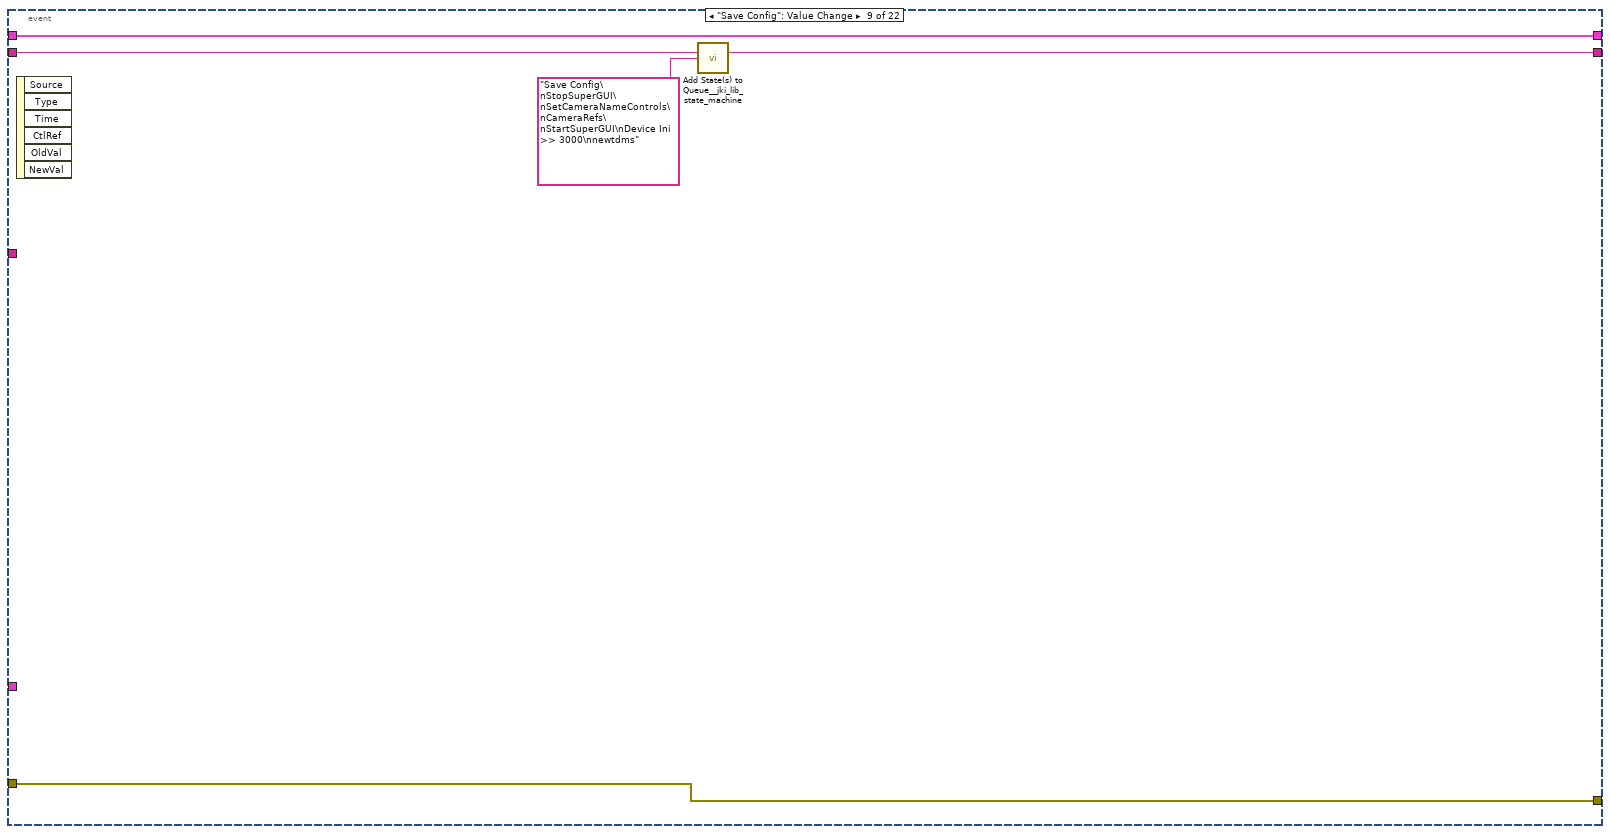
[diagram p19: hidden frame]
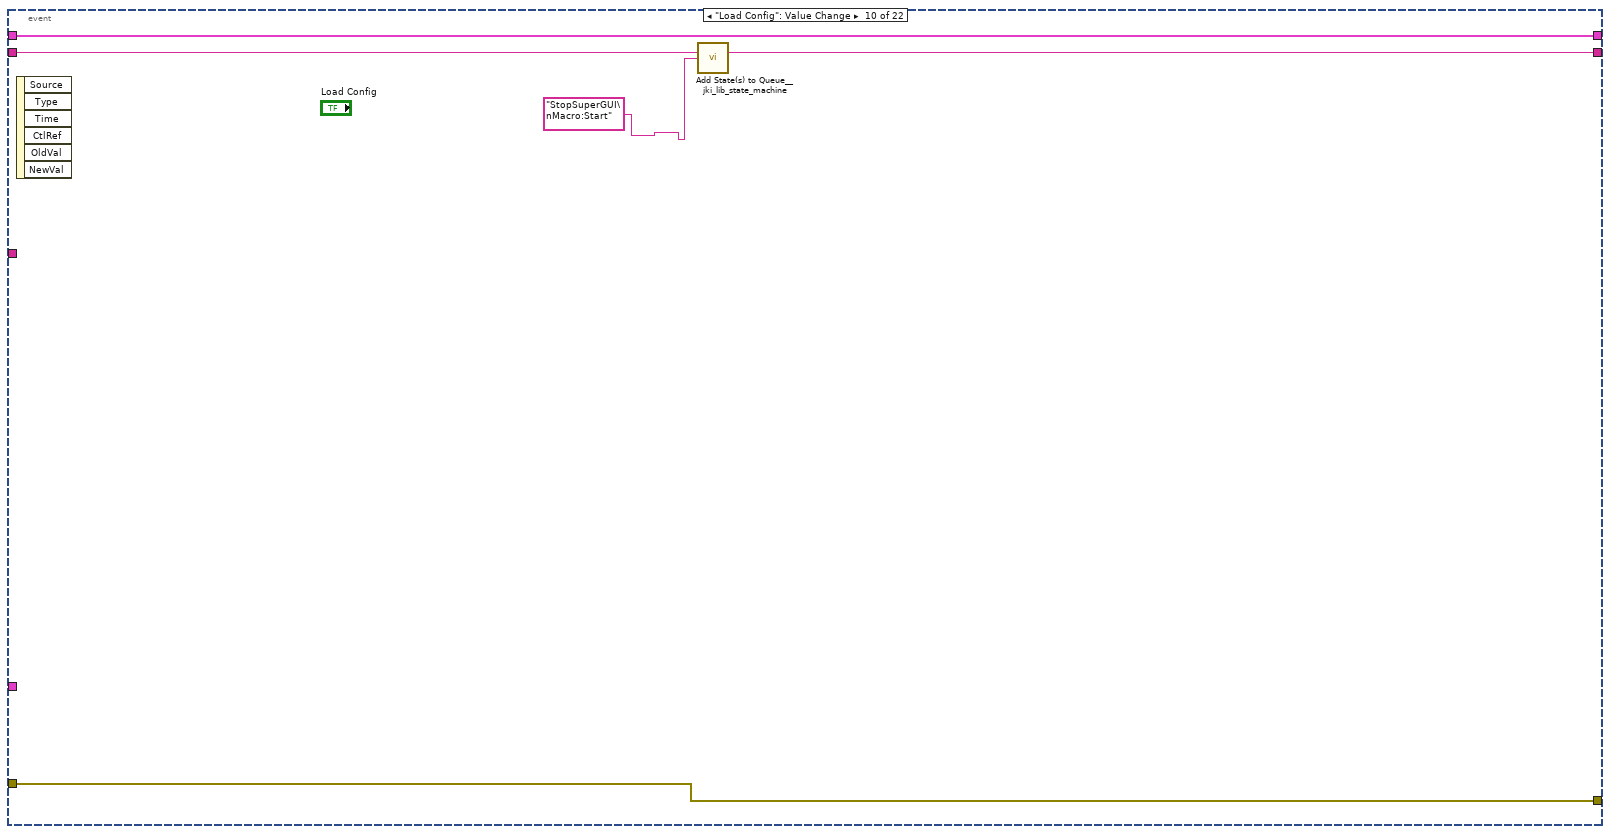
[diagram p20: hidden frame]
diagram:
  (unwired) T11 {"Tolerance [%]"=0.1, "Stepsize"=0.0001, "Invert Direction X"=FALSE, "Invert Direction Y"=TRUE, "enable feedback"=FALSE, "Set Centriod Target"=FALSE, "xCal"=0.0001, "xCal neg"=0.0001, "yCal"=0.0001, "yCal neg"=0.0001} ("move config  2")
  # "Motor Config"
  # "Load Config\nSetCameraNameControls\nCameraRefs\nStartSuperGUI\nDevice Ini >> 3000\nnewtdms"
  # "StopSuperGUI\nMacro:Start"
  # "why device ini every time in timeout? after a move, should reset img average"
  n1 = Tick Count (ms)() -> (millisecond timer value=→"millisecond timer value":u32)
  n2 = control-ref of="Target.X::1"() -> (w43:refnum<vi>)
  n3 = control-ref of="Target.Y::1"() -> (w42:refnum<vi>)
  n4 = control-ref of="Target.X::2"() -> (w41:refnum<vi>)
  n5 = control-ref of="Target.Y::2"() -> (w40:refnum<vi>)
  n6 = control-ref of="Target.X::3"() -> (w39:refnum<vi>)
  n7 = control-ref of="Target.Y::3"() -> (w38:refnum<vi>)
  n8 = control-ref of="Target.X::4"() -> (w37:refnum<vi>)
  n9 = control-ref of="Target.Y::4"() -> (w36:refnum<vi>)
  n10 = control-ref of="Target.X::5"() -> (w35:refnum<vi>)
  n11 = control-ref of="Target.Y::5"() -> (w34:refnum<vi>)
  n12 = control-ref of="Target.X::6"() -> (w33:refnum<vi>)
  n13 = control-ref of="Target.Y::6"() -> (w32:refnum<vi>)
  n14 = control-ref of="Target.X::7"() -> (w31:refnum<vi>)
  n15 = control-ref of="Target.Y::7"() -> (w30:refnum<vi>)
  n16 = control-ref of="Target.X::8"() -> (w29:refnum<vi>)
  n17 = control-ref of="Target.Y::8"() -> (w28:refnum<vi>)
  n18 = control-ref of="Target.X::9"() -> (w14:refnum<vi>)
  n19 = control-ref of="Target.Y::9"() -> (w13:refnum<vi>)
  n20 = control-ref of="Target.X::10"() -> (w12:refnum<vi>)
  n21 = control-ref of="Target.Y::10"() -> (w11:refnum<vi>)
  n22 = control-ref of="Target.X::11"() -> (w10:refnum<vi>)
  n23 = control-ref of="Target.Y::11"() -> (w9:refnum<vi>)
  n24 = control-ref of="Target.X::12"() -> (w8:refnum<vi>)
  n25 = control-ref of="Target.Y::12"() -> (w7:refnum<vi>)
  n26 = Bundle("Target.X::1"=w43, "Target.Y::1"=w42) -> (w27:T12)  [unwired: 1 in]
  n27 = Bundle("Target.X::2"=w41, "Target.Y::2"=w40) -> (w26:T13)  [unwired: 1 in]
  n28 = Bundle("Target.X::3"=w39, "Target.Y::3"=w38) -> (w25:T14)  [unwired: 1 in]
  n29 = Bundle("Target.X::4"=w37, "Target.Y::4"=w36) -> (w18:T15)  [unwired: 1 in]
  n30 = Bundle("Target.X::5"=w35, "Target.Y::5"=w34) -> (w24:T16)  [unwired: 1 in]
  n31 = Bundle("Target.X::6"=w33, "Target.Y::6"=w32) -> (w23:T17)  [unwired: 1 in]
  n32 = Bundle("Target.X::7"=w31, "Target.Y::7"=w30) -> (w22:T18)  [unwired: 1 in]
  n33 = Bundle("Target.X::8"=w29, "Target.Y::8"=w28) -> (w21:T19)  [unwired: 1 in]
  n34 = Bundle("Target.X::12"=w8, "Target.Y::12"=w7) -> (w3:T20)  [unwired: 1 in]
  n35 = Bundle("Target.X::9"=w14, "Target.Y::9"=w13) -> (w6:T21)  [unwired: 1 in]
  n36 = Bundle("Target.X::10"=w12, "Target.Y::10"=w11) -> (w5:T22)  [unwired: 1 in]
  n37 = Bundle("Target.X::11"=w10, "Target.Y::11"=w9) -> (w4:T23)  [unwired: 1 in]
  n38 = disable-structure shown="Disabled" {
    frame Disabled {
    }
    frame Enabled {
    }
  }
  n39 = Build Array(w27, w26, w25, w18, w24, w23, w22, w21, w6, w5, w4, w3) -> (w20:T24)
  n40 = property on="Feedback Global" class="Bool (strict)"("Value"=FALSE ("Feedback Global")) -> ()  [unwired: 2 in, 2 out]
  n41 = call <vilib>:"Add State(s) to Queue__jki_lib_state_machine.vi"("State(s) in (\"\")"="Macro: Initialize") -> ("States Out"=w47:string)  [unwired: 14 in]
  n42 = while "JKI - String-Based Queued State Machine (Basic) v1.0" {
    shift-right: [w62] -> w17
    shift-left: _ -> [w56]
    shift-right: [w64] -> w44
    shift-left: _ -> [w61]
    shift-right: [w50] -> _
    shift-left: w47 -> [w65]
    tunnel: w20 -> [w59]
    tunnel: [w51] -> w45
    tunnel: w20 -> [w58]
    stop <- w63 stop-if-true
    n43 = Unbundle By Name(w56) -> ("active cams"=w55:string[], "Mean Centroid X"=w54:dbl[][], "Mean Centroid Y"=w53:dbl[][], "Mean Size"=w52:dbl[][])
    n44 = call <vilib>:"Parse State Queue__jki_lib_state_machine.vi"("State Queue"=w65, "Error In (no error)"=w61) -> ("Remaining States"=w67:string, "Current State"=w48:string, "Arguments"=w66:string)  [unwired: 11 in]
    "Current State" <- w48
    n45 = local read "CCDs"() -> (w51:string[])
    n46 = case shown="\"\", \"Idle\"" w48 {
      selector: w48 -> [_ _ w403 _ _ _ _ _ _ _ _ _ _ _ _ _ _ _ _ _ _ _ _ _ _ _ _ _ _ _ _ _ _ _ _ _ _ _ _ _ _ _ _ _ _ _ _ _ _ _ _ _]
      tunnel: w67 -> [w133 w401 w407 w426 w433 w439 w444 w482 w494 w502 w512 w517 w524 w536 w561 w567 w610 w620 w628 w640 w645 w678 w739 w757 w787 w808 w836 w917 w965 w993 w1005 w1038 w1048 w1053 w1075 w1221 w1387 w1446 w1491 w1539 w1581 w1625 w1630 w1637 w1713 w1762 w1773 w1793 w1890 w1917 w1933 w1955]
      tunnel: w66 -> [_ _ _ _ _ _ _ _ _ _ _ _ w519 w531 _ _ _ _ _ _ _ w655 _ _ _ _ w814 _ w954 _ _ _ _ _ w1076 _ w1378 w1436 w1481 w1528 w1575 _ _ _ _ _ _ _ _ _ _ _]
      tunnel: w56 -> [w131 w398 w405 w416 w430 w437 w441 _ w487 w499 w509 w515 w522 w530 w558 w564 w570 w616 w625 w632 w642 w648 w737 w755 w785 w793 w829 w915 w951 w989 w1002 w1031 w1042 w1050 w1064 w1204 w1372 w1427 w1470 w1523 w1577 w1618 w1627 w1634 w1709 w1759 w1770 w1789 w1888 w1914 w1935 w1946]
      tunnel: [w130 w399 w409 w424 errorcluster {"status"=FALSE, "code"=0, "source"=""} ("error out") w436 w442 w456 w492 w498 w510 w514 w520 w533 w559 w565 w608 w618 w626 w638 w643 w651 w736 w754 w784 w790 w832 w913 w956 w991 w994 w1036 w1046 w1051 w1104 w1234 w1368 w1444 w1489 w1518 w1573 w1623 w1628 w1635 w1710 w1760 w1771 w1782 w1859 w1915 w1931 w1953] -> w64
      tunnel: w61 -> [w129 w399 w408 w424 w427 w436 w442 w456 w484 w498 w510 w514 w521 w534 w559 w565 w608 w618 w626 w638 w643 w649 w736 w754 w784 w791 w833 w914 w940 w991 w995 w1036 w1046 w1051 w1104 w1234 w1367 w1444 w1489 w1517 w1574 w1623 w1628 w1635 w1711 w1760 w1771 w1783 w1886 w1915 w1931 w1953]
      tunnel: [w132 w400 w406 w425 w432 w438 w443 w481 w493 w501 w511 w516 w523 w535 w560 w566 w609 w619 w627 w639 w644 w677 w738 w756 w786 w807 w823 w916 w964 w992 w1004 w1037 w1047 w1052 w1058 w1235 w1386 w1445 w1490 w1538 w1580 w1624 w1629 w1636 w1712 w1761 w1772 w1792 w1889 w1916 w1932 w1954] -> w50
      tunnel: [_ _ _ _ _ TRUE _ _ _ _ _ _ _ _ _ _ _ _ _ _ _ _ _ _ _ _ _ _ _ _ _ _ _ _ _ _ _ _ _ _ _ _ _ _ _ _ _ _ _ _ _ _] -> w63
      tunnel: [w126 w398 w405 w415 w430 w437 w441 w457 w487 w499 w509 w515 w522 w530 w558 w564 w569 w615 w625 w632 w642 w670 w737 w755 w785 w792 w834 w915 w959 w988 w1003 w1030 w1041 w1050 w1057 w1205 w1371 w1426 w1469 w1522 w1579 w1617 w1627 w1634 w1709 w1758 w1770 w1789 w1887 w1914 w1934 w1945] -> w62
      tunnel: "update speed [ms]" -> [w128 _ _ _ _ _ _ _ _ _ _ _ _ _ _ _ _ _ _ _ _ _ _ _ _ _ _ _ _ _ _ _ _ _ _ _ _ _ _ _ _ _ _ _ _ _ _ _ _ _ _ _]
      tunnel: w59 -> [w125 _ _ _ _ _ _ _ _ _ _ _ _ _ _ _ _ _ _ _ _ _ _ _ _ _ _ _ _ _ _ _ _ _ w1055 _ _ _ _ _ _ _ _ _ _ _ _ _ _ w1899 _ _]
      tunnel: w51 -> [w127 _ _ _ _ _ _ _ _ _ _ _ _ _ _ _ _ _ _ _ _ _ _ _ _ _ w835 _ w960 _ _ _ _ _ w1068 w1206 w1385 _ _ w1537 w1576 _ _ w1633 _ _ _ w1788 _ _ _ _]
      tunnel: [w124 w397 w402 w414 w428 w434 w440 w449 w490 w495 w508 w513 w518 w529 w557 w562 w607 w611 w623 w629 w641 w660 w735 w740 w758 w788 w810 w900 w949 w984 w998 w1029 w1040 w1049 w1056 w1195 w1376 w1435 w1480 w1527 w1572 w1622 w1626 w1631 w1691 w1753 w1769 w1774 w1860 w1897 w1927 w1936] -> w49
      tunnel: w48 -> [w124 w397 w402 w414 w428 w434 w440 w449 w490 w495 w508 w513 w518 w529 w557 w562 w607 w611 w623 w629 w641 w660 w735 w740 w758 w788 w810 w900 w949 w984 w998 w1029 w1040 w1049 w1056 w1195 w1376 w1435 w1480 w1527 w1572 w1622 w1626 w1631 w1691 w1753 w1769 w1774 w1860 w1897 w1927 w1936]
      frame "", "Idle" {
        # "executes when the state queue is empty"
        n47 = event shown="[10] \"Load Config 2\": Value Change" {
          selector: _ -> [_ _ _ _ _ _ _ _ _ _ _ _ _ _ _ _ _ _ _ _ _ _]
          dyn-events: _ -> [_ _ _ _ _ _ _ _ _ _ _ _ _ _ _ _ _ _ _ _ _ _]
          timeout: w128 -> [_ _ _ _ _ _ _ _ _ _ _ _ _ _ _ _ _ _ _ _ _ _]
          tunnel: w133 -> [w152 w219 w234 w259 w264 w269 w274 w280 w285 w290 w318 w323 w325 w340 w352 w357 w362 w368 w376 w385 w389 w396]
          tunnel: [w163 w218 w233 w258 w263 w268 w273 w279 w284 w289 w317 w322 w324 w339 w351 w356 w361 w367 w375 w384 w388 w395] -> w132
          tunnel: w131 -> [w141 w216 w231 w255 w261 w266 w271 w277 w282 w287 w315 w320 w328 w338 w350 w355 w360 w366 w374 w378 w390 w393]
          tunnel: [w169 w217 w232 w257 w262 w267 w272 w278 w283 w288 w316 w321 w327 w333 w345 w354 w359 w365 w373 w383 w387 w394] -> w130
          tunnel: w129 -> [w159 w217 w232 w257 w262 w267 w272 w278 w283 w288 w316 w321 w327 w334 w346 w354 w359 w365 w373 w383 w387 w394]
          tunnel: [w145 w216 w231 w254 w261 w266 w271 w277 w282 w287 w315 w320 w328 w338 w350 w355 w360 w366 w374 w378 w390 w393] -> w126
          tunnel: w127 -> [w160 _ w227 _ _ _ _ _ _ _ _ _ _ _ _ _ _ _ _ _ _ _]
          tunnel: w125 -> [_ _ w229 _ _ _ _ _ _ _ _ _ _ _ _ _ _ _ _ _ _ _]
          event Timeout {
            n48 = event-data() -> ()  [unwired: 1 in, 1 out]
            n49 = Unbundle By Name(w141) -> ("Detection.img to avg"=w150:i32)
            n50 = Unbundle By Name(w141) -> ("active ccd"=w147:i32)
            n51 = Unbundle By Name(w141) -> ("Detection"=w148:T32, "active cams"=w143:string[])
            n52 = Increment(x=w150) -> (x+1=w164:i32)
            n53 = Array Size(array=w143) -> (size(s)=w142:i32)
            n54 = Greater Or Equal?(x="#imgs avd so far", y=w164) -> (x >= y?=w162:bool)
            n55 = Increment(x="#imgs avd so far") -> (x+1=w166:dbl)
            n56 = call "centroid detection loop.vi"("CCDs"=w160, "error in (no error)"=w159, "active cams"=w143, "Detection in"=w148, "autodetect"="autodetect") -> ("error out"=w157:errorcluster, "# where centr y is 0"=w155:i32[], "Detection out"=w144:T33, "bounding rectangle"=→"Box":T2, "detected array"=→"detected":bool[], "Particle Reports (Pixels)"=w158:T34)  [unwired: 1 in]
            n57 = Equal To 0?(x=w142) -> ()  [unwired: 1 out]
            n58 = Select(t=0.0, s=w162, f=w166) -> (s? t:f=w165:dbl)
            n59 = Unbundle By Name(w141) -> ("Config loaded"=w140:bool)
            n60 = Index Array(array=w158, index (row)=w147) -> (element=w135:T6)  [unwired: 1 in]
            n61 = for {
              tunnel: w135 -> [w175] mode=indexing
              tunnel: [w174] -> w139 mode=indexing
              n62 = Unbundle By Name(w175) -> ("Area"=w174:dbl)
            }
            n63 = call-poly <userlib>:"Sort Array__ogtk.vi"("Order"=enum16{"ascending", "descending"}."descending", "Array in"=w139) -> ("Sorted Pointers"=w137:i32[])  [unwired: 8 in, 1 out]
            n64 = call-poly <userlib>:"Reorder Array2__ogtk.vi"("indices"=w137, "array"=w135) -> ("reordered array"=w136:variant[])  [unwired: 9 in]
            n65 = local write "#imgs avd so far"(w165) -> ()
            n66 = Variant To Data(type=w135, Variant=w136) -> (data=→"active ccd particles":T6)  [unwired: 1 in, 1 out]
            n67 = call <vilib>:"Clear Errors.vi"("error in (no error)"=w157) -> ("error out"=w169:errorcluster)  [unwired: 5 in, 1 out]
            n68 = Unbundle By Name(w144) -> ("img to avg"=w153:i32)
            n69 = for {
              tunnel: w155 -> [w208] mode=indexing
              tunnel: w143 -> [w214] mode=indexing
              shift-right: [w209] -> w170
              shift-left: "" ("GUIdevice 7") -> [w212]
              tunnel: [w203] -> w172 mode=indexing
              tunnel: "Detection Rate" -> [w207]
              tunnel: w165 -> [w205]
              tunnel: w150 -> [w201]
              # "averaging done?"
              n70 = Greater Or Equal?(x=w208, y=w201) -> (x >= y?=w204:bool)
              n71 = Multiply(x=w207, y=w205) -> (x*y=w206:dbl)
              n72 = Greater Or Equal?(x=w208, y=w206) -> (x >= y?=w202:bool)
              n73 = And(x=w204, y=w202) -> (x .and. y?=w203:bool)
              n74 = Select(t=w214, s=w203, f="") -> (s? t:f=w210:string)
              n75 = Concatenate Strings(w212, "\t", w210) -> (w209:string)
            }
            n76 = case shown="True" w140 {
              tunnel: w152 -> [w176 w179]
              tunnel: [w176 w178] -> w151
              frame False {
              }
              frame True {
                n77 = call <vilib>:"Add State(s) to Queue__jki_lib_state_machine.vi"("State(s) in (\"\")"=w179, "State(s) at Back (\"\")"="Device Ini" ("State(s) at Back (\"\")")) -> ("States Out"=w178:string)  [unwired: 13 in]
              }
            }
            n78 = case shown="True" w162 {
              tunnel: w144 -> [w180 w187]
              tunnel: [w180 w186] -> w146
              tunnel: w153 -> [_ w182]
              frame False {
              }
              frame True {
                # "avg done. clear arrays"
                n79 = Decrement(x=w182) -> (x-1=w185:i32)
                n80 = Initialize Array(0.0 ("element"), 12 ("dimension size"), w185) -> (w181:dbl[][])
                n81 = Bundle By Name(cluster=w187, "Centroid X"=w181, "Centroid Y"=w181, "Size"=w181) -> (w186:T33)
              }
            }
            n82 = Bundle By Name(cluster=w141, "Detection"=w146) -> (w145:T35)
            n83 = Or Array Elements(Boolean array=w172) -> (logical OR=w171:bool)
            n84 = case shown="True" w171 {
              tunnel: w170 -> [_ w195]
              tunnel: w151 -> [w188 w194]
              tunnel: [w188 w189] -> w163
              frame False {
                # "avg not done yet"
              }
              frame True {
                # "avg done."
                n85 = local read "Tab Cams"() -> (w192:T3)
                n86 = call <vilib>:"Build State String with Arguments__jki_lib_state_machine.vi"("Arguments (\"\")"=w195, "State"="detected") -> ("State with Arguments"=w193:string)  [unwired: 4 in]
                n87 = call <vilib>:"Add State(s) to Queue__jki_lib_state_machine.vi"("State(s) in Front (\"\")"=w193, "State(s) in (\"\")"=w194) -> ("States Out"=w190:string)  [unwired: 13 in]
                n88 = case shown="Default" w192 {
                  tunnel: w190 -> [w197 w200]
                  tunnel: "stats" ("State") -> [_ w199]
                  tunnel: [w197 w198] -> w189
                  frame Default {
                  }
                  frame "History" {
                    n89 = call <vilib>:"Add State(s) to Queue__jki_lib_state_machine.vi"("State(s) in Front (\"\")"=w199, "State(s) in (\"\")"=w200) -> ("States Out"=w198:string)  [unwired: 13 in]
                  }
                }
              }
            }
          }
          event "stop": Value Change {
            # "Exit Button Value Change (pressed) Event\n(this executes Macro: Exit to terminate the VI)"
            n90 = event-data() -> ()  [unwired: 1 in, 6 out]
            n91 = call <vilib>:"Add State(s) to Queue__jki_lib_state_machine.vi"("State(s) in Front (\"\")"="Macro: Exit", "State(s) in (\"\")"=w219) -> ("States Out"=w218:string)  [unwired: 13 in]
          }
          event Value Change {
            n92 = event-data() -> ()  [unwired: 1 in, 6 out]
            n93 = Unbundle By Name(w231) -> ("active ccd"=w223:i32, "Mean Centroid X"=w222:dbl[][], "Mean Centroid Y"=w221:dbl[][])
            n94 = Index Array(array=w227, index=w223) -> (element=w226:string)
            n95 = Concatenate Strings("Do want to update the target of " ("message"), w226, "?" ("string")) -> (w224:string)
            n96 = property on="Set Centriod Target" class="Bool (strict)"("Value"=FALSE) -> ()  [unwired: 2 in, 2 out]
            n97 = Two Button Dialog(message=w224) -> (T button?=w230:bool)  [unwired: 2 in]
            n98 = case shown="True" w230 {
              tunnel: w229 -> [_ w243]
              tunnel: w223 -> [_ w242]
              tunnel: w222 -> [_ w249]
              tunnel: w221 -> [_ w244]
              frame False {
              }
              frame True {
                n99 = Index Array(array=w249, index (row)=w242) -> (element=w248:dbl[])  [unwired: 1 in]
                n100 = Index Array(array=w244, index (row)=w242) -> (element=w245:dbl[])  [unwired: 1 in]
                n101 = Index Array(array=w243, index=w242) -> (element=w241:T20)
                n102 = Unbundle By Name(w241) -> ("Target.X::12"=w240:refnum<vi>, "Target.Y::12"=w239:refnum<vi>)
                n103 = Reverse 1D Array(array=w248) -> (reversed array=w247:dbl[])
                n104 = Reverse 1D Array(array=w245) -> (reversed array=w246:dbl[])
                n105 = Index Array(array=w247) -> (element=w238:dbl)  [unwired: 1 in]
                n106 = Index Array(array=w246) -> (element=w236:dbl)  [unwired: 1 in]
                n107 = To Unsigned Word Integer(number=w236) -> (unsigned 16bit integer=w235:u16)
                n108 = To Unsigned Word Integer(number=w238) -> (unsigned 16bit integer=w237:u16)
                n109 = disable-structure shown="Enabled" {
                  disable-tunnel: w240 -> [w253 _]
                  disable-tunnel: w237 -> [w252 _]
                  disable-tunnel: w239 -> [w251 _]
                  disable-tunnel: w235 -> [w250 _]
                  frame Enabled {
                    n110 = property class="DigNum (strict)"(reference=w253, "Val(Sgnl)"=w252) -> ()  [unwired: 1 in, 2 out]
                    n111 = property class="DigNum (strict)"(reference=w251, "Val(Sgnl)"=w250) -> ()  [unwired: 1 in, 2 out]
                  }
                  frame Disabled {
                  }
                }
              }
            }
            n112 = call <vilib>:"Add State(s) to Queue__jki_lib_state_machine.vi"("State(s) in (\"\")"=w234) -> ("States Out"=w233:string)  [unwired: 14 in]
          }
          event "Feedback Global": Value Change {
            # "Exit Button Value Change (pressed) Event\n(this executes Macro: Exit to terminate the VI)"
            n113 = event-data() -> ("NewVal"=w256:bool)  [unwired: 1 in, 5 out]
            n114 = call <vilib>:"Add State(s) to Queue__jki_lib_state_machine.vi"("State(s) in (\"\")"=w259) -> ("States Out"=w258:string)  [unwired: 14 in]
            n115 = Bundle By Name(cluster=w255, "Feedback global"=w256) -> (w254:T35)
          }
          event Value Change {
            n116 = event-data() -> ()  [unwired: 1 in, 6 out]
            n117 = call <vilib>:"Add State(s) to Queue__jki_lib_state_machine.vi"("State(s) in Front (\"\")"="set move props from control", "State(s) in (\"\")"=w264) -> ("States Out"=w263:string)  [unwired: 13 in]
          }
          event Value Change {
            n118 = event-data() -> ()  [unwired: 1 in, 6 out]
            n119 = call <vilib>:"Add State(s) to Queue__jki_lib_state_machine.vi"("State(s) in Front (\"\")"="set detection params from control", "State(s) in (\"\")"=w269) -> ("States Out"=w268:string)  [unwired: 13 in]
          }
          event Value Change {
            n120 = event-data() -> ()  [unwired: 1 in, 6 out]
            n121 = call <vilib>:"Add State(s) to Queue__jki_lib_state_machine.vi"("State(s) in Front (\"\")"="set thresholds", "State(s) in (\"\")"=w274) -> ("States Out"=w273:string)  [unwired: 13 in]
          }
          event "Reset History": Value Change {
            n122 = event-data() -> ()  [unwired: 1 in, 6 out]
            n123 = call <vilib>:"Add State(s) to Queue__jki_lib_state_machine.vi"("State(s) in (\"\")"=w280, "State(s) at Back (\"\")"="Reset History" ("State(s) at Back (\"\")")) -> ("States Out"=w279:string)  [unwired: 13 in]
            n124 = property on="Reset History" class="Bool (strict)"("Value"=FALSE ("Reset History")) -> ()  [unwired: 2 in, 2 out]
          }
          event "Save Config": Value Change {
            n125 = event-data() -> ()  [unwired: 1 in, 6 out]
            n126 = call <vilib>:"Add State(s) to Queue__jki_lib_state_machine.vi"("State(s) in (\"\")"=w285, "State(s) at Back (\"\")"="Save Config\nStopSuperGUI\nSetCameraNameControls\nCameraRefs\nStartSuperGUI\nDevice Ini >> 3000\nnewtdms" ("State(s) at Back (\"\")")) -> ("States Out"=w284:string)  [unwired: 13 in]
          }
          event "Load Config": Value Change {
            n127 = event-data() -> ()  [unwired: 1 in, 6 out]
            n128 = call <vilib>:"Add State(s) to Queue__jki_lib_state_machine.vi"("State(s) in (\"\")"=w290, "State(s) at Back (\"\")"="StopSuperGUI\nMacro:Start" ("State(s) at Back (\"\")")) -> ("States Out"=w289:string)  [unwired: 13 in]
          }
          event "Load Config 2": Value Change {
            n129 = event-data() -> ()  [unwired: 1 in, 6 out]
            n130 = Unbundle By Name(w315) -> ("dev var alias arrays.dev variable alias Motors X"=w308:string[][], "dev var alias arrays.dev variable alias Motors Y"=w309:string[][], "move properties"=w310:T11[])  [unwired: 2 out]
            n131 = Index Array(array=w308, index (row)="downstream mirror") -> ()  [unwired: 1 in, 1 out]
            n132 = Index Array(array=w309, index (row)="downstream mirror") -> ()  [unwired: 1 in, 1 out]
            n133 = Index Array(array=w310, index="downstream mirror") -> (element=w306:T11)
            n134 = Index Array(array=w308, index (row)="upstream mirror") -> (element=w313:string[])  [unwired: 1 in]
            n135 = Index Array(array=w309, index (row)="upstream mirror") -> ()  [unwired: 1 in, 1 out]
            n136 = Index Array(array=w310, index="upstream mirror") -> (element=w311:T11)
            n137 = Unbundle By Name(w311) -> ("xCal"=w300:dbl, "yCal"=w297:dbl)  [unwired: 2 out]
            n138 = Unbundle By Name(w306) -> ("xCal"=w301:dbl, "yCal"=w296:dbl)  [unwired: 2 out]
            n139 = call <vilib>:"Add State(s) to Queue__jki_lib_state_machine.vi"("State(s) in (\"\")"=w318) -> ("States Out"=w317:string)  [unwired: 14 in]
            n140 = call "coupled mirror calibration.vi"("seperation"="seperation", "distance to target plane"="distance to target plane", "pixel calib"="pixel calib", "xCal 2"=w301, "xCal"=w300, "x'"="x'", "x"="x") -> ("A2x"=→"A2x":dbl, "A1x"=→"A1x":dbl)  [unwired: 3 in]
            n141 = call "coupled mirror calibration.vi"("seperation"="seperation", "distance to target plane"="distance to target plane", "pixel calib"="pixel calib", "xCal 2"=w296, "xCal"=w297, "x'"="y'", "x"="y") -> ("A2x"=→"A2y":dbl, "A1x"=→"A1y":dbl)  [unwired: 3 in]
            n142 = call "get set udp value from dev var alias array.vi"("get or set"=enum16{"get", "set"}."get", "dev variable alias Motors X"=w313) -> ()  [unwired: 8 in, 2 out]
          }
          event "Save Stats": Value Change {
            n143 = event-data() -> ()  [unwired: 1 in, 6 out]
            n144 = call <vilib>:"Add State(s) to Queue__jki_lib_state_machine.vi"("State(s) in (\"\")"=w323, "State(s) at Back (\"\")"="Save Stats" ("State(s) at Back (\"\")")) -> ("States Out"=w322:string)  [unwired: 13 in]
          }
          event "Tab Cams": Value Change {
            n145 = event-data() -> ()  [unwired: 1 in, 6 out]
            n146 = call <vilib>:"Add State(s) to Queue__jki_lib_state_machine.vi"("State(s) in (\"\")"=w325, "State(s) at Back (\"\")"="stats" ("State")) -> ("States Out"=w324:string)  [unwired: 13 in]
          }
          event "Left", "Right": Value Change {
            n147 = event-data() -> ("CtlRef"=w337:refnum<vi>)  [unwired: 1 in, 5 out]
            n148 = property class="Bool (strict)"(reference=w337, error in=w334) -> (reference out=w336:refnum<vi>, error out=w335:errorcluster, "Label.Text"=w331:string)
            n149 = property class="Bool (strict)"(reference=w336, error in=w335, "Value"=FALSE) -> (error out=w333:errorcluster)  [unwired: 1 out]
            n150 = call <vilib>:"Build State String with Arguments__jki_lib_state_machine.vi"("Arguments (\"\")"=w331, "State"="ManMove X") -> ("State with Arguments"=w330:string)  [unwired: 4 in]
            n151 = call <vilib>:"Add State(s) to Queue__jki_lib_state_machine.vi"("State(s) in (\"\")"=w340, "State(s) at Back (\"\")"=w330) -> ("States Out"=w339:string)  [unwired: 13 in]
          }
          event "Up", "Down": Value Change {
            n152 = event-data() -> ("CtlRef"=w349:refnum<vi>)  [unwired: 1 in, 5 out]
            n153 = property class="Bool (strict)"(reference=w349, error in=w346) -> (reference out=w348:refnum<vi>, error out=w347:errorcluster, "Label.Text"=w343:string)
            n154 = property class="Bool (strict)"(reference=w348, error in=w347, "Value"=FALSE) -> (error out=w345:errorcluster)  [unwired: 1 out]
            n155 = call <vilib>:"Build State String with Arguments__jki_lib_state_machine.vi"("Arguments (\"\")"=w343, "State"="ManMove Y") -> ("State with Arguments"=w342:string)  [unwired: 4 in]
            n156 = call <vilib>:"Add State(s) to Queue__jki_lib_state_machine.vi"("State(s) in (\"\")"=w352, "State(s) at Back (\"\")"=w342) -> ("States Out"=w351:string)  [unwired: 13 in]
          }
          event "Center": Value Change {
            n157 = event-data() -> ()  [unwired: 1 in, 6 out]
            n158 = call <vilib>:"Add State(s) to Queue__jki_lib_state_machine.vi"("State(s) in (\"\")"=w357, "State(s) at Back (\"\")"="Center" ("State(s) at Back (\"\")")) -> ("States Out"=w356:string)  [unwired: 13 in]
          }
          event "new tdms", "tdms root": Value Change {
            n159 = event-data() -> ()  [unwired: 1 in, 6 out]
            n160 = call <vilib>:"Add State(s) to Queue__jki_lib_state_machine.vi"("State(s) in (\"\")"=w362, "State(s) at Back (\"\")"="newtdms" ("State(s) at Back (\"\")")) -> ("States Out"=w361:string)  [unwired: 13 in]
          }
          event "device ini": Value Change {
            n161 = event-data() -> ()  [unwired: 1 in, 6 out]
            n162 = property on="device ini" class="Bool (strict)"("Value"=FALSE ("test")) -> ()  [unwired: 2 in, 2 out]
            n163 = disable-structure shown="Enabled" {
              disable-tunnel: ["Device Ini" ("State(s) at Back (\"\")") "StopSuperGUI\nMacro:Start" ("State(s) at Back (\"\")")] -> w364
              frame Disabled {
              }
              frame Enabled {
              }
            }
            n164 = call <vilib>:"Add State(s) to Queue__jki_lib_state_machine.vi"("State(s) in (\"\")"=w368, "State(s) at Back (\"\")"=w364) -> ("States Out"=w367:string)  [unwired: 13 in]
          }
          event "clear error": Value Change {
            n165 = event-data() -> ()  [unwired: 1 in, 6 out]
            n166 = property on="clear error" class="Bool (strict)"("Value"=FALSE ("test")) -> ()  [unwired: 2 in, 2 out]
            n167 = local write "error out"(errorcluster {"status"=FALSE, "code"=0, "source"=""} ("error out")) -> ()
            n168 = call <vilib>:"Add State(s) to Queue__jki_lib_state_machine.vi"("State(s) in (\"\")"=w376) -> ("States Out"=w375:string)  [unwired: 14 in]
          }
          event "active CCDs": Value Change {
            n169 = event-data() -> ("NewVal"=w379:i32)  [unwired: 1 in, 5 out]
            n170 = Unbundle By Name(w378) -> ("active cams"=w380:string[])
            n171 = Index Array(array=w380, index=w379) -> (element=w381:string)
            n172 = call <vilib>:"Build State String with Arguments__jki_lib_state_machine.vi"("Arguments (\"\")"=w381, "State"="active" ("State(s) at Back (\"\")")) -> ("State with Arguments"=w377:string)  [unwired: 4 in]
            n173 = call <vilib>:"Add State(s) to Queue__jki_lib_state_machine.vi"("State(s) in (\"\")"=w385, "State(s) at Back (\"\")"=w377) -> ("States Out"=w384:string)  [unwired: 13 in]
          }
          event "img to avg": Value Change {
            n174 = event-data() -> ()  [unwired: 1 in, 6 out]
            n175 = call <vilib>:"Add State(s) to Queue__jki_lib_state_machine.vi"("State(s) in Front (\"\")"="ImgToAvg" ("State(s) at Back (\"\")"), "State(s) in (\"\")"=w389) -> ("States Out"=w388:string)  [unwired: 13 in]
          }
          event Panel Close? {
            # "Discard the event because we'll close the front panel ourselves in Macro: Exit"
            # "Close Panel button (pressed) Event\n(this executes Macro: Exit to terminate the VI)"
            n176 = event-data() -> ()  [unwired: 1 in, 1 out]
            n177 = call <vilib>:"Add State(s) to Queue__jki_lib_state_machine.vi"("State(s) in Front (\"\")"="Macro: Exit", "State(s) in (\"\")"=w396) -> ("States Out"=w395:string)  [unwired: 13 in]
            n178 = event-data("Discard?"=TRUE) -> ()  [unwired: 1 in, 1 out]
          }
        }
      }
      frame "---------- Core ----------" {
        # "Do not put any code in this frame.\n(it is a separator no-op)"
        n179 = call <vilib>:"Add State(s) to Queue__jki_lib_state_machine.vi"("State(s) in (\"\")"=w401) -> ("States Out"=w400:string)  [unwired: 14 in]
      }
      frame Default {
        w412 = 42 items=["No error", "Argument error", "Memory is full", "Out of zone", "End of file", "File already open", "Generic file I/O error", "File not found", "File permission error", "Disk is full", "Duplicate path", "Too many files open", "System feature not enabled", "Resource file not found", "Cannot add resource", "Resource not found", "Image not found", "Image memory error", "Pen does not exist", "Config type invalid", "Config token not found", "Config parse error", "Config memory error", "Bad external code format", "Bad external code offset", "External code not present", "Null window", "Destroy window error", "Null menu", "Print aborted", "Bad print record", "Print driver error", "Windows error during printing", "Memory error during printing", "Print dialog error", "Generic print error", "Invalid device refnum", "Device not found", "Device parameter error", "Device unit error", "Cannot open device", "Device call aborted", "Generic error", "Cancelled by user", "Object ID too low", "Object ID too high", "Object not in heap", "Unknown heap", "Unknown object (invalid DefProc)", "Unknown object (DefProc not in table)", "Message out of range", "Invalid (null) method", "Unknown message", "Manager call not supported", "Bad address", "Network operation in progress", "Network operation timed out", "Connection is busy", "Network attribute not supported", "Network error", "Address in use", "System out of memory", "Connection aborted", "Connection refused", "Not connected", "Already connected", "Connection closed", "Initialization error (interapplication manager)", "Bad occurrence", "Wait on unbound occurrence handler", "Occurrence queue overflow", "Datalog type conflict", "Unused", "Unrecognized type (interapplication manager)", "Memory corrupt", "Failed to make temporary DLL", "Old CIN version", "Drag socket not found", "Failed to load drop-object", "Failed to register OLE object", "Failed to release OLE object", "Format specifier type mismatch", "Unknown format specifier", "Too few format specifiers", "Too many format specifiers", "Scan failed", "Newer CIN version", "Error converting to variant", "Runtime menu error", "Password tampered", "Variant attribute not found", "Incompatible variant data type", "Event data is not available", "Event Store is not present", "Occurrence is not found", "Event Queue is not created", "Event info is not available", "Refnum passed is NULL", "Error retrieving Class GUID", "Error retrieving CoClass GUID", "Error retrieving TypeLib GUID.", "Bad built application magic bytes.", "Specific driver is different from the specific driver associated with the Logical Name.", "There is no session opened to the class driver.", "Max Error", "MAX - Error with config objects", "MAX - Error loading configuration", "MAX - Group not supported"]
        # "Current State"
        # "Do not delete, rename, or modify this frame.\n(this is used to capture unhandled states and typos)"
        # "Handle mistyped state name (developer tool)"
        n180 = Format Into String(format string="Software Exception: Unhandled State \"%s\"." ("message"), error in=w408, w403) -> (resulting string=w411:string, error out=w410:errorcluster)  [unwired: 1 in]
        n181 = call <vilib>:"Error Cluster From Error Code.vi"("show call chain? (False)"=TRUE, "error in (no error)"=w410, "error message (\"\")"=w411, "error code (0)"=w412) -> ("error out"=w409:errorcluster)  [unwired: 5 in]
        n182 = call <vilib>:"Add State(s) to Queue__jki_lib_state_machine.vi"("State(s) in (\"\")"=w407) -> ("States Out"=w406:string)  [unwired: 14 in]
      }
      frame "Initialize Core Data" {
        # "Do not delete, rename, or modify this frame.\n(this is used to determine panel behavior on exit)"
        # "originally closed?"
        # "exe?"
        # "If panel starts closed or is an EXE, then close it when we exit"
        n183 = property class="VI"() -> ("Front Panel.Open"=w423:bool)  [unwired: 2 in, 2 out]
        n184 = property class="App"() -> ("App.Kind"=w422:T25)  [unwired: 2 in, 2 out]
        n185 = control-ref of="Current VI Reference"() -> (w417:refnum<vi>)
        n186 = Not(x=w423) -> (.not. x?=w420:bool)
        n187 = Equal?(x=w422, y=T25."Run Time System" ("Application:Kind")) -> (x = y?=w419:bool)
        n188 = Or(x=w420, y=w419) -> (x .or. y?=w418:bool)
        n189 = Bundle By Name(cluster=w416, "Core.Current VI Reference"=w417, "Core.Close Panel on Exit?"=w418) -> (w415:T35)
        n190 = call <vilib>:"Add State(s) to Queue__jki_lib_state_machine.vi"("State(s) in (\"\")"=w426) -> ("States Out"=w425:string)  [unwired: 14 in]
      }
      frame "Error Handler" {
        # "Unhandled Error -- Display it"
        # "Handle any errors here.\nYou can also output any states to clean-up after errors occur"
        # "Clear error"
        n191 = call <vilib>:"Add State(s) to Queue__jki_lib_state_machine.vi"("State(s) in Front (\"\")"="/* Post Error States", "State(s) in (\"\")"=w433) -> ("States Out"=w432:string)  [unwired: 13 in]
        "error out" <- w427
      }
      frame "Exit" {
        # "Do not put any code in this frame.\n(No errors that occur here will be handled.)"
        n192 = call <vilib>:"Add State(s) to Queue__jki_lib_state_machine.vi"("State(s) in (\"\")"=w439) -> ("States Out"=w438:string)  [unwired: 14 in]
      }
      frame "---------- Data ----------" {
        # "Do not put any code in this frame.\n(It is a separator no-op. You can make a copy of this frame to create a new Data frame)"
        n193 = call <vilib>:"Add State(s) to Queue__jki_lib_state_machine.vi"("State(s) in (\"\")"=w444) -> ("States Out"=w443:string)  [unwired: 14 in]
      }
      frame "Data: Initialize" {
        w445 = FALSE  # Config loaded
        w447 = T32 {"detection para"=[{"Filter"=1, "Filter Para"={"X Size"=5, "Y Size"=5, "% Tolerance"=1}, "detection method"=4, "Particle filtering"=[{"Measurement Parameter"=35, "Range Lower Value"=0.0, "Range Upper Value"=0.0, "Range"=TRUE, "Measurement Type"=FALSE}], "Remove small Objects"=TRUE, "Restrict to round Objects"=FALSE, "Use Cam COM"=FALSE}, {"Filter"=1, "Filter Para"={"X Size"=5, "Y Size"=5, "% Tolerance"=1}, "detection method"=4, "Particle filtering"=[{"Measurement Parameter"=35, "Range Lower Value"=0.0, "Range Upper Value"=500.0, "Range"=FALSE, "Measurement Type"=FALSE}], "Remove small Objects"=TRUE, "Restrict to round Objects"=FALSE, "Use Cam COM"=FALSE}, {"Filter"=1, "Filter Para"={"X Size"=5, "Y Size"=5, "% Tolerance"=1}, "detection method"=4, "Particle filtering"=[{"Measurement Parameter"=35, "Range Lower Value"=0.0, "Range Upper Value"=500.0, "Range"=TRUE, "Measurement Type"=FALSE}], "Remove small Objects"=TRUE, "Restrict to round Objects"=FALSE, "Use Cam COM"=FALSE}, {"Filter"=1, "Filter Para"={"X Size"=5, "Y Size"=5, "% Tolerance"=1}, "detection method"=4, "Particle filtering"=[{"Measurement Parameter"=35, "Range Lower Value"=0.0, "Range Upper Value"=500.0, "Range"=TRUE, "Measurement Type"=FALSE}], "Remove small Objects"=TRUE, "Restrict to round Objects"=FALSE, "Use Cam COM"=FALSE}, {"Filter"=1, "Filter Para"={"X Size"=5, "Y Size"=5, "% Tolerance"=1}, "detection method"=4, "Particle filtering"=[{"Measurement Parameter"=35, "Range Lower Value"=0.0, "Range Upper Value"=500.0, "Range"=TRUE, "Measurement Type"=FALSE}], "Remove small Objects"=TRUE, "Restrict to round Objects"=FALSE, "Use Cam COM"=FALSE}, {"Filter"=1, "Filter Para"={"X Size"=5, "Y Size"=5, "% Tolerance"=1}, "detection method"=4, "Particle filtering"=[{"Measurement Parameter"=35, "Range Lower Value"=0.0, "Range Upper Value"=500.0, "Range"=TRUE, "Measurement Type"=FALSE}], "Remove small Objects"=TRUE, "Restrict to round Objects"=FALSE, "Use Cam COM"=FALSE}, {"Filter"=1, "Filter Para"={"X Size"=5, "Y Size"=5, "% Tolerance"=1}, "detection method"=4, "Particle filtering"=[{"Measurement Parameter"=35, "Range Lower Value"=0.0, "Range Upper Value"=500.0, "Range"=TRUE, "Measurement Type"=FALSE}], "Remove small Objects"=TRUE, "Restrict to round Objects"=FALSE, "Use Cam COM"=FALSE}, {"Filter"=1, "Filter Para"={"X Size"=5, "Y Size"=5, "% Tolerance"=1}, "detection method"=3, "Particle filtering"=[{"Measurement Parameter"=35, "Range Lower Value"=0.0, "Range Upper Value"=0.0, "Range"=FALSE, "Measurement Type"=FALSE}], "Remove small Objects"=TRUE, "Restrict to round Objects"=FALSE, "Use Cam COM"=FALSE}, {"Filter"=1, "Filter Para"={"X Size"=5, "Y Size"=5, "% Tolerance"=1}, "detection method"=4, "Particle filtering"=[{"Measurement Parameter"=35, "Range Lower Value"=0.0, "Range Upper Value"=0.0, "Range"=FALSE, "Measurement Type"=FALSE}], "Remove small Objects"=TRUE, "Restrict to round Objects"=FALSE, "Use Cam COM"=FALSE}, {"Filter"=1, "Filter Para"={"X Size"=5, "Y Size"=5, "% Tolerance"=1}, "detection method"=4, "Particle filtering"=[{"Measurement Parameter"=35, "Range Lower Value"=0.0, "Range Upper Value"=500.0, "Range"=TRUE, "Measurement Type"=FALSE}], "Remove small Objects"=TRUE, "Restrict to round Objects"=FALSE, "Use Cam COM"=FALSE}, {"Filter"=1, "Filter Para"={"X Size"=5, "Y Size"=5, "% Tolerance"=1}, "detection method"=4, "Particle filtering"=[{"Measurement Parameter"=35, "Range Lower Value"=0.0, "Range Upper Value"=500.0, "Range"=TRUE, "Measurement Type"=FALSE}], "Remove small Objects"=TRUE, "Restrict to round Objects"=FALSE, "Use Cam COM"=FALSE}, {"Filter"=1, "Filter Para"={"X Size"=5, "Y Size"=5, "% Tolerance"=1}, "detection method"=4, "Particle filtering"=[{"Measurement Parameter"=35, "Range Lower Value"=0.0, "Range Upper Value"=500.0, "Range"=TRUE, "Measurement Type"=FALSE}], "Remove small Objects"=TRUE, "Restrict to round Objects"=FALSE, "Use Cam COM"=FALSE}], "thresholds"=[{"Lower value"=93.0, "Upper value"=255.0}, {"Lower value"=105.0, "Upper value"=255.0}, {"Lower value"=0.0, "Upper value"=255.0}, {"Lower value"=127.0, "Upper value"=255.0}, {"Lower value"=0.0, "Upper value"=255.0}, {"Lower value"=0.0, "Upper value"=255.0}, {"Lower value"=0.0, "Upper value"=255.0}, {"Lower value"=0.0, "Upper value"=255.0}, {"Lower value"=0.0, "Upper value"=255.0}, {"Lower value"=0.0, "Upper value"=255.0}, {"Lower value"=0.0, "Upper value"=255.0}, {"Lower value"=0.0, "Upper value"=255.0}], "Centroid X"=[], "Centroid Y"=[], "Size"=[], "Centroid refs"=[], "img to avg"=6}  # Detection
        w448 = T36 {"Positions x"=[0.0, 0.0, 0.0, 0.0, 0.0, 0.0, 0.0, 0.0, 0.0, 0.0, 0.0, 0.0], "Positions y"=[0.0, 0.0, 0.0, 0.0, 0.0, 0.0, 0.0, 0.0, 0.0, 0.0, 0.0, 0.0]}  # Motor positions
        w450 = T37 {"dev variable alias"=[], "dev variable alias Motors X"=[], "dev variable alias Motors Y"=[]}  # dev var alias arrays
        w468 = dbl[][] []  # Offset Y stats
        w476 = dbl[][] []  # Mean Size
        w474 = T11[] [{"Tolerance [%]"=0.1, "Stepsize"=0.0001, "Invert Direction X"=FALSE, "Invert Direction Y"=TRUE, "enable feedback"=FALSE, "Set Centriod Target"=FALSE, "xCal"=0.0001, "xCal neg"=0.0001, "yCal"=0.0001, "yCal neg"=0.0001}, {"Tolerance [%]"=0.1, "Stepsize"=0.0001, "Invert Direction X"=FALSE, "Invert Direction Y"=TRUE, "enable feedback"=FALSE, "Set Centriod Target"=FALSE, "xCal"=0.0001, "xCal neg"=0.0001, "yCal"=0.0001, "yCal neg"=0.0001}, {"Tolerance [%]"=0.1, "Stepsize"=0.0001, "Invert Direction X"=FALSE, "Invert Direction Y"=TRUE, "enable feedback"=FALSE, "Set Centriod Target"=FALSE, "xCal"=0.0001, "xCal neg"=0.0001, "yCal"=0.0001, "yCal neg"=0.0001}, {"Tolerance [%]"=0.1, "Stepsize"=0.0001, "Invert Direction X"=FALSE, "Invert Direction Y"=TRUE, "enable feedback"=FALSE, "Set Centriod Target"=FALSE, "xCal"=0.0001, "xCal neg"=0.0001, "yCal"=0.0001, "yCal neg"=0.0001}, {"Tolerance [%]"=0.1, "Stepsize"=0.0001, "Invert Direction X"=FALSE, "Invert Direction Y"=TRUE, "enable feedback"=FALSE, "Set Centriod Target"=FALSE, "xCal"=0.0001, "xCal neg"=0.0001, "yCal"=0.0001, "yCal neg"=0.0001}, {"Tolerance [%]"=0.1, "Stepsize"=0.0001, "Invert Direction X"=FALSE, "Invert Direction Y"=TRUE, "enable feedback"=FALSE, "Set Centriod Target"=FALSE, "xCal"=0.0001, "xCal neg"=0.0001, "yCal"=0.0001, "yCal neg"=0.0001}, {"Tolerance [%]"=0.1, "Stepsize"=0.0001, "Invert Direction X"=FALSE, "Invert Direction Y"=TRUE, "enable feedback"=FALSE, "Set Centriod Target"=FALSE, "xCal"=0.0001, "xCal neg"=0.0001, "yCal"=0.0001, "yCal neg"=0.0001}, {"Tolerance [%]"=0.1, "Stepsize"=0.0001, "Invert Direction X"=FALSE, "Invert Direction Y"=TRUE, "enable feedback"=FALSE, "Set Centriod Target"=FALSE, "xCal"=0.0001, "xCal neg"=0.0001, "yCal"=0.0001, "yCal neg"=0.0001}, {"Tolerance [%]"=0.1, "Stepsize"=0.0001, "Invert Direction X"=FALSE, "Invert Direction Y"=TRUE, "enable feedback"=FALSE, "Set Centriod Target"=FALSE, "xCal"=0.0001, "xCal neg"=0.0001, "yCal"=0.0001, "yCal neg"=0.0001}, {"Tolerance [%]"=0.1, "Stepsize"=0.0001, "Invert Direction X"=FALSE, "Invert Direction Y"=TRUE, "enable feedback"=FALSE, "Set Centriod Target"=FALSE, "xCal"=0.0001, "xCal neg"=0.0001, "yCal"=0.0001, "yCal neg"=0.0001}, {"Tolerance [%]"=0.1, "Stepsize"=0.0001, "Invert Direction X"=FALSE, "Invert Direction Y"=TRUE, "enable feedback"=FALSE, "Set Centriod Target"=FALSE, "xCal"=0.0001, "xCal neg"=0.0001, "yCal"=0.0001, "yCal neg"=0.0001}, {"Tolerance [%]"=0.1, "Stepsize"=0.0001, "Invert Direction X"=FALSE, "Invert Direction Y"=TRUE, "enable feedback"=FALSE, "Set Centriod Target"=FALSE, "xCal"=0.0001, "xCal neg"=0.0001, "yCal"=0.0001, "yCal neg"=0.0001}, {"Tolerance [%]"=0.1, "Stepsize"=0.0001, "Invert Direction X"=FALSE, "Invert Direction Y"=TRUE, "enable feedback"=FALSE, "Set Centriod Target"=FALSE, "xCal"=0.0001, "xCal neg"=0.0001, "yCal"=0.0001, "yCal neg"=0.0001}]  # move properties
        w473 = T38 []  # active axis refs 2
        w467 = dbl[][] []  # Motor X
        w466 = dbl[][] []  # Motor Y
        w465 = string[] []  # active cams
        w451 = T39 {"STOP queue"=refnum, "SuperGUI ref"=refnum}  # Supergui
        w452 = dbl[] [0.0, 0.0, 0.0, 0.0, 0.0, 0.0, 0.0, 0.0, 0.0, 0.0, 0.0, 0.0]  # steps speed Y
        w453 = dbl[] [0.0, 0.0, 0.0, 0.0, 0.0, 0.0, 0.0, 0.0, 0.0, 0.0, 0.0, 0.0]  # steps speed X
        w454 = refnum<k34> refnum  # tdms ref
        w455 = bool[] [FALSE, FALSE, FALSE, FALSE, TRUE, TRUE, TRUE, FALSE, FALSE, FALSE, FALSE, FALSE]  # detected
        w462 = bool[] [FALSE, FALSE, FALSE, FALSE, FALSE, FALSE, FALSE, FALSE, FALSE, FALSE, FALSE, TRUE]  # speedmode Y
        w463 = bool[] [FALSE, FALSE, FALSE, FALSE, FALSE, FALSE, FALSE, FALSE, FALSE, FALSE, FALSE, TRUE]  # speedmode X
        w471 = FALSE  # Feedback global
        w472 = 0  # active ccd
        w480 = T40 {"Current VI Reference"=refnum, "Close Panel on Exit?"=FALSE}  # Core
        # "Initialize the shift-register data, here.\n(data names are defined by what you wire into the bundle function)"
        n194 = call <vilib>:"Add State(s) to Queue__jki_lib_state_machine.vi"("State(s) in (\"\")"=w482) -> ("States Out"=w481:string)  [unwired: 14 in]
        n195 = Unbundle By Name(w447) -> ("img to avg"=w446:i32)
        n196 = Bundle("Core"=w480, "Detection"=w447, "Mean Centroid X"="Mean Centroid X", "Mean Centroid Y"=dbl[][] [], "Offset X"="Offset X", "Offset Y"=dbl[][] [], "Offset X stats"=dbl[][] [], "Offset Y stats"=w468, "Mean Size"=w476, "Time"="Time", "move properties"=w474, "active axis refs 2"=w473, "active ccd"=w472, "Feedback global"=w471, "Motor X"=w467, "Motor Y"=w466, "active cams"=w465, "tdms ref"=w454, "active man refs"="active man refs", "detected"=w455, "speedmode X"=w463, "speedmode Y"=w462, "steps speed X"=w453, "steps speed Y"=w452, "Supergui"=w451, "dev var alias arrays"=w450, "Motor positions"=w448, "Config loaded"=w445) -> (w458:T35)  [unwired: 1 in]
        n197 = Initialize Array(0.0 ("element"), 12 ("dimension size"), w446) -> (w461:dbl[][])
        n198 = Bundle By Name(cluster=w458, "Detection.Centroid X"=w461, "Detection.Centroid Y"=w461, "Detection.Size"=w461) -> (w457:T35)
      }
      frame "Data: Cleanup" {
        # "Cleanup any data and references, here.\n(this is called automatically, by the Macro: Exit)"
        n199 = Unbundle By Name(w487) -> ("Core.Current VI Reference"=w491:refnum<vi>)
        n200 = Unbundle By Name(w487) -> ("tdms ref"=w489:refnum<k34>)
        n201 = call "close fgv udp connections.vi"("error in"=w484) -> ("error out"=w483:errorcluster)  [unwired: 10 in]
        n202 = TDMS Close(8:w483, 11:w489) -> (0:w488:errorcluster)  [unwired: 1 out]
        n203 = call <vilib>:"Clear Errors.vi"("error in (no error)"=w488) -> ("error out"=w486:errorcluster)  [unwired: 5 in, 1 out]
        n204 = Merge Errors(w486, w483) -> (w485:errorcluster)
        n205 = Close Reference(reference=w491, error in (no error)=w485) -> (error out=w492:errorcluster)
        n206 = call <vilib>:"Add State(s) to Queue__jki_lib_state_machine.vi"("State(s) in (\"\")"=w494) -> ("States Out"=w493:string)  [unwired: 14 in]
      }
      frame "StopSuperGUI" {
        # "Initialize the User Interface, here.\n(this is called automatically, by the Macro: Init)"
        n207 = Unbundle By Name(w499) -> ("Supergui.SuperGUI ref"=w497:refnum<vi>, "Supergui.STOP queue"=w500:refnum<queue>)
        n208 = Not A Number/Path/Refnum?(number/path/refnum=w497) -> (NaN/Path/Refnum?=w496:bool)
        n209 = case shown="False" w496 {
          tunnel: w500 -> [w507 _]
          tunnel: w497 -> [w503 _]
          frame False {
            n210 = Release Queue(queue=w507) -> (error out=w506:errorcluster)  [unwired: 2 in, 2 out]
            n211 = call-by-ref "Wait On Asynchronous Call"(reference=w503, error in=w506) -> (error out=w505:errorcluster, 0:"error out"=w504:errorcluster)  [unwired: 11 in, 1 out]
            n212 = call <vilib>:"Clear Errors.vi"("error in (no error)"=w504) -> ()  [unwired: 5 in, 2 out]
            n213 = call <vilib>:"Clear Errors.vi"("error in (no error)"=w505) -> ()  [unwired: 5 in, 2 out]
          }
          frame True {
          }
        }
        n214 = call <vilib>:"Add State(s) to Queue__jki_lib_state_machine.vi"("State(s) in (\"\")"=w502) -> ("States Out"=w501:string)  [unwired: 14 in]
      }
      frame "---------- UI ----------" {
        # "Do not put any code in this frame.\n(It is a separator no-op. You can make a copy of this frame to create a new UI frame)"
        n215 = call <vilib>:"Add State(s) to Queue__jki_lib_state_machine.vi"("State(s) in (\"\")"=w512) -> ("States Out"=w511:string)  [unwired: 14 in]
      }
      frame "UI: Initialize" {
        # "Initialize the User Interface, here.\n(this is called automatically, by the Macro: Init)"
        n216 = call <vilib>:"Add State(s) to Queue__jki_lib_state_machine.vi"("State(s) in (\"\")"=w517) -> ("States Out"=w516:string)  [unwired: 14 in]
      }
      frame "UI: Cursor Set" {
        # "Argument"
        # "Set and Unset Cursor Busy.\n(Usage: \"UI: Cursor Set >> Busy|Idle\")"
        n217 = case shown="\"Idle\", Default" w519 {
          tunnel: w521 -> [w526 w528]
          tunnel: [w525 w527] -> w520
          frame "Idle", Default {
            n218 = call <vilib>:"Unset Busy.vi"("error in (no error)"=w526) -> ("error out"=w525:errorcluster)  [unwired: 10 in]
          }
          frame "Busy" {
            n219 = call <vilib>:"Set Busy.vi"("error in (no error)"=w528) -> ("error out"=w527:errorcluster)  [unwired: 9 in, 1 out]
          }
        }
        n220 = call <vilib>:"Add State(s) to Queue__jki_lib_state_machine.vi"("State(s) in (\"\")"=w524) -> ("States Out"=w523:string)  [unwired: 14 in]
      }
      frame "UI: Front Panel State" {
        # "Argument"
        # "Set Front Panel Open or Closed\n(Usage: \"UI: Front Panel State >> Open|Close\")"
        n221 = Unbundle By Name(w530) -> ("Core.Current VI Reference"=w532:refnum<vi>)
        n222 = case shown="\"Open\", Default" w531 {
          tunnel: w534 -> [w540 w551]
          tunnel: [w541 w552] -> w533
          tunnel: w532 -> [_ _]
          frame "Open", Default {
            n223 = property class="VI"(error in=w540) -> (reference out=w538:refnum<vi>, error out=w539:errorcluster, "Front Panel.Open"=w537:bool)  [unwired: 1 in]
            n224 = case shown="False" w537 {
              tunnel: [w544 w547] -> w541
              tunnel: w539 -> [w543 w547]
              tunnel: w538 -> [w542 _]
              frame False {
                n225 = invoke class="VI" method="FP.Open"(reference=w542, error in=w543, "Activate"=TRUE, "State"=T26."Standard") -> (error out=w544:errorcluster)  [unwired: 1 in, 4 out]
              }
              frame True {
              }
            }
          }
          frame "Close" {
            n226 = property class="VI"(error in=w551) -> (reference out=w549:refnum<vi>, error out=w550:errorcluster, "Front Panel.Open"=w548:bool)  [unwired: 1 in]
            n227 = case shown="True" w548 {
              tunnel: [w553 w556] -> w552
              tunnel: w550 -> [w553 w555]
              tunnel: w549 -> [_ w554]
              frame False {
              }
              frame True {
                n228 = invoke class="VI" method="FP.Close"(reference=w554, error in=w555) -> (error out=w556:errorcluster)  [unwired: 1 in, 2 out]
              }
            }
          }
        }
        n229 = call <vilib>:"Add State(s) to Queue__jki_lib_state_machine.vi"("State(s) in (\"\")"=w536) -> ("States Out"=w535:string)  [unwired: 14 in]
      }
      frame "---------- Macro ----------" {
        # "Do not put any code in this frame.\n(It is a separator no-op. You can make a copy of this frame to create a new Macro frame)"
        n230 = call <vilib>:"Add State(s) to Queue__jki_lib_state_machine.vi"("State(s) in (\"\")"=w561) -> ("States Out"=w560:string)  [unwired: 14 in]
      }
      frame "Macro: Initialize" {
        # "Initialization Macro\n(This is called once, when the VI starts)"
        n231 = call <vilib>:"Add State(s) to Queue__jki_lib_state_machine.vi"("State(s) in Front (\"\")"="Data: Initialize\nCentroidRefs\nInitialize Core Data\nUI: Initialize\nUI: Front Panel State >> Open\nGetMotorsFromDB\nMacro:Start", "State(s) in (\"\")"=w567) -> ("States Out"=w566:string)  [unwired: 13 in]
      }
      frame "CentroidRefs" {
        n232 = control-ref of="centroidx::1"() -> (w606:refnum<vi>)
        n233 = control-ref of="centroidy::1"() -> (w605:refnum<vi>)
        n234 = control-ref of="centroidx::2"() -> (w604:refnum<vi>)
        n235 = control-ref of="centroidy::2"() -> (w603:refnum<vi>)
        n236 = control-ref of="centroidx::3"() -> (w602:refnum<vi>)
        n237 = control-ref of="centroidy::3"() -> (w601:refnum<vi>)
        n238 = control-ref of="centroidx::4"() -> (w600:refnum<vi>)
        n239 = control-ref of="centroidy::4"() -> (w599:refnum<vi>)
        n240 = control-ref of="centroidx::5"() -> (w598:refnum<vi>)
        n241 = control-ref of="centroidy::5"() -> (w597:refnum<vi>)
        n242 = control-ref of="centroidx::6"() -> (w596:refnum<vi>)
        n243 = control-ref of="centroidy::6"() -> (w595:refnum<vi>)
        n244 = control-ref of="centroidx::7"() -> (w594:refnum<vi>)
        n245 = control-ref of="centroidy::7"() -> (w593:refnum<vi>)
        n246 = control-ref of="centroidx::8"() -> (w592:refnum<vi>)
        n247 = control-ref of="centroidy::8"() -> (w591:refnum<vi>)
        n248 = control-ref of="centroidx::9"() -> (w582:refnum<vi>)
        n249 = control-ref of="centroidy::9"() -> (w581:refnum<vi>)
        n250 = control-ref of="centroidx::10"() -> (w580:refnum<vi>)
        n251 = control-ref of="centroidy::10"() -> (w579:refnum<vi>)
        n252 = control-ref of="centroidx::11"() -> (w578:refnum<vi>)
        n253 = control-ref of="centroidy::11"() -> (w577:refnum<vi>)
        n254 = control-ref of="centroidx::12"() -> (w576:refnum<vi>)
        n255 = control-ref of="centroidy::12"() -> (w575:refnum<vi>)
        n256 = Bundle("centroidx::1"=w606, "centroidy::1"=w605) -> (w590:T41)  [unwired: 1 in]
        n257 = Bundle("centroidx::2"=w604, "centroidy::2"=w603) -> (w589:T42)  [unwired: 1 in]
        n258 = Bundle("centroidx::3"=w602, "centroidy::3"=w601) -> (w588:T43)  [unwired: 1 in]
        n259 = Bundle("centroidx::4"=w600, "centroidy::4"=w599) -> (w583:T44)  [unwired: 1 in]
        n260 = Bundle("centroidx::5"=w598, "centroidy::5"=w597) -> (w587:T45)  [unwired: 1 in]
        n261 = Bundle("centroidx::6"=w596, "centroidy::6"=w595) -> (w586:T46)  [unwired: 1 in]
        n262 = Bundle("centroidx::7"=w594, "centroidy::7"=w593) -> (w585:T47)  [unwired: 1 in]
        n263 = Bundle("centroidx::8"=w592, "centroidy::8"=w591) -> (w584:T48)  [unwired: 1 in]
        n264 = Bundle("centroidx::12"=w576, "centroidy::12"=w575) -> (w571:T49)  [unwired: 1 in]
        n265 = Bundle("centroidx::9"=w582, "centroidy::9"=w581) -> (w574:T50)  [unwired: 1 in]
        n266 = Bundle("centroidx::10"=w580, "centroidy::10"=w579) -> (w573:T51)  [unwired: 1 in]
        n267 = Bundle("centroidx::11"=w578, "centroidy::11"=w577) -> (w572:T52)  [unwired: 1 in]
        n268 = Build Array(w590, w589, w588, w583, w587, w586, w585, w584, w574, w573, w572, w571) -> (w568:T53)
        n269 = Bundle By Name(cluster=w570, "Detection.Centroid refs"=w568) -> (w569:T35)
        n270 = call <vilib>:"Add State(s) to Queue__jki_lib_state_machine.vi"("State(s) in (\"\")"=w610) -> ("States Out"=w609:string)  [unwired: 14 in]
      }
      frame "GetMotorsFromDB" {
        n271 = call "get all aliases of a class.vi"("class (eg motor)"="motor") -> ("dev variable alias"=w614:string[][])  [unwired: 10 in]
        n272 = Bundle By Name(cluster=w616, "dev var alias arrays.dev variable alias"=w614) -> (w615:T35)
        n273 = Index Array(array=w614, index (col)=2 ("disabled index (col)")) -> (element=w612:string[])  [unwired: 1 in]
        "Names" <- w612
        n274 = property on="Motor Alias Y" class="Ring (strict)"("Strings []"=w612) -> ()  [unwired: 2 in, 2 out]
        n275 = property on="Motor Alias X" class="Ring (strict)"("Strings []"=w612) -> ()  [unwired: 2 in, 2 out]
        n276 = call <vilib>:"Add State(s) to Queue__jki_lib_state_machine.vi"("State(s) in (\"\")"=w620) -> ("States Out"=w619:string)  [unwired: 14 in]
      }
      frame "Macro:Start" {
        # "Initialization Macro\n(This is called once, when the VI starts)"
        n277 = local write "config path"("" ("config path")) -> ()
        n278 = call <vilib>:"Add State(s) to Queue__jki_lib_state_machine.vi"("State(s) in Front (\"\")"="Load Config\nSetCameraNameControls\nCameraRefs\nStartSuperGUI\nDevice Ini >> 3000\nnewtdms\nImgToAvg", "State(s) in (\"\")"=w628) -> ("States Out"=w627:string)  [unwired: 13 in]
        n279 = local write "active CCDs"(0 ("active CCDs")) -> ()
      }
      frame "Macro: Exit" {
        # "Exit Macro\n(This is called once, when the VI exits)"
        n280 = Unbundle By Name(w632) -> ("Core.Close Panel on Exit?"=w631:bool)
        n281 = Select(t="UI: Front Panel State >> Close", s=w631, f="") -> (s? t:f=w635:string)
        n282 = call <vilib>:"Add State(s) to Queue__jki_lib_state_machine.vi"("State(s) in Front (\"\")"="StopSuperGUI" ("State(s) in Front (\"\")"), "State(s) in (\"\")"=w635, "State(s) at Back (\"\")"="Data: Cleanup\nExit") -> ("States Out"=w633:string)  [unwired: 12 in]
        n283 = call <vilib>:"Add State(s) to Queue__jki_lib_state_machine.vi"("State(s) in Front (\"\")"=w633, "State(s) in (\"\")"=w640) -> ("States Out"=w639:string)  [unwired: 13 in]
      }
      frame "---------- Ini and Configure ----------" {
        # "Template Separator\n(You can make a copy of, or modify, this frame)"
        n284 = call <vilib>:"Add State(s) to Queue__jki_lib_state_machine.vi"("State(s) in (\"\")"=w645) -> ("States Out"=w644:string)  [unwired: 14 in]
      }
      frame "Load Config" {
        w662 = T54 {"Camera"="", "Motor Alias X"=0, "Motor Alias Y"=0}  # Camera and motors
        # "Your code here.\n(You can make a copy of, or modify, this frame)"
        n285 = Unbundle By Name(w648) -> ("Detection.detection para"=w676:T8[], "move properties"=w673:T11[], "Detection.thresholds"=w668:cluster{"Lower value":sgl, "Upper value":sgl}[])
        n286 = Empty String/Path?(string/path=w655) -> (empty?=w656:bool)
        n287 = case shown="True" w656 {
          tunnel: [w694 w703] -> w652
          tunnel: w649 -> [w693 w702]
          tunnel: [w693 w701] -> w653
          tunnel: w655 -> [w695 _]
          frame False {
            n288 = String To Path(string=w695) -> (path=w694:path)
          }
          frame True {
            n289 = call <vilib>:"Application Directory.vi"() -> ("Application Directory"=w697:path)
            n290 = Build Path(base path=w697, name or relative path=path "cfg") -> (appended path=w699:path)
            n291 = call-poly <userlib>:"File Exists__ogtk.vi"("file path"=w699) -> ("exists"=w698:bool)  [unwired: 6 in, 1 out]
            n292 = case shown="True" w698 {
              tunnel: w699 -> [w707 w708]
              tunnel: [w706 w708] -> w696
              frame False {
                n293 = Create Folder(path (use dialog)=w707) -> (created path=w706:path)  [unwired: 2 in, 2 out]
              }
              frame True {
              }
            }
            n294 = call "File Dialog2"("start path"=w696, "error in"=w702, "pattern (all files)"="*.cfg", "pattern label"="config") -> ("selected path"=w703:path, "error out"=w701:errorcluster)  [unwired: 8 in, 2 out]
          }
        }
        n295 = property on="Load Config" class="Bool (strict)"("Value"=FALSE ("Load Config")) -> ()  [unwired: 2 in, 2 out]
        n296 = case shown="No Error" w653 {
          tunnel: w678 -> [w689 _]
          tunnel: [w688 _] -> w677
          tunnel: w653 -> [w683 _]
          tunnel: w652 -> [w682 _]
          tunnel: [w681 w692] -> w651
          tunnel: [w680 T27 {"Camera names"=[], "Motor aliases x"=[], "Motor aliases y"=[], "detection para"=[], "thresholds"=[], "move properties"=[], "tdms root"=path "c:/BP_DATAsd"} ("BP Configuration")] -> w650
          tunnel: w649 -> [_ w692]
          tunnel: [TRUE ("Config loaded") FALSE ("Config loaded")] -> w646
          frame No Error {
            w684 = T27 {"Camera names"=[], "Motor aliases x"=[], "Motor aliases y"=[], "detection para"=[], "thresholds"=[], "move properties"=[], "tdms root"=path "c:/BP_DATAsd"}  # BP Configuration
            n297 = call <userlib>:"MGI Read Anything.vi"("Type of Anything"=w684, "Error In"=w683, "Path (dialog)"=w682) -> ("Error Out"=w686:errorcluster, "Anything"=w685:variant)  [unwired: 5 in, 2 out]
            n298 = Variant To Data(error in=w686, type=w684, Variant=w685) -> (data=w680:T27, error out=w681:errorcluster)
            n299 = call <vilib>:"Add State(s) to Queue__jki_lib_state_machine.vi"("State(s) in (\"\")"=w689, "State(s) at Back (\"\")"="Motor Config" ("State(s) at Back (\"\")")) -> ("States Out"=w688:string)  [unwired: 13 in]
          }
          frame Error {
          }
        }
        n300 = Path To String(path=w652) -> (string=→"config path":string)
        n301 = Unbundle By Name(w650) -> ("Motor aliases x"=w667:string[], "Motor aliases y"=w664:string[], "Camera names"=w659:string[], "detection para"=w675:T8[], "move properties"=w674:T11[], "thresholds"=w669:cluster{"Lower value":sgl, "Upper value":sgl}[], "tdms root"=w654:path)
        n302 = local write "tdms root"(w654) -> ()
        n303 = Bundle By Name(cluster=w648, "Config loaded"=w646) -> (w647:T35)
        n304 = call-poly <userlib>:"Remove Duplicates from 1D Array__ogtk.vi"("Input Array"=w659) -> ("Output Array"=w658:string[])  [unwired: 1 out]
        "CCDs" <- w658
        n305 = property on="Motor Alias X" class="Ring (strict)"() -> ("Strings []"=w663:string[])  [unwired: 2 in, 2 out]
        n306 = for {
          tunnel: w658 -> [w731]
          tunnel: w675 -> [w733]
          tunnel: w674 -> [w732]
          shift-right: [w726] -> w672
          shift-left: w676 -> [w730]
          shift-right: [w724] -> w671
          shift-left: w673 -> [w729]
          tunnel: w669 -> [w725]
          shift-right: [w721] -> w665
          shift-left: w668 -> [w723]
          tunnel: w667 -> [w720]
          tunnel: w664 -> [w718]
          tunnel: w663 -> [w714]
          tunnel: w662 -> [w716]
          tunnel: [w711] -> w661 mode=indexing
          tunnel: w658 -> [w709] mode=indexing
          i -> [w719]
          n307 = call-poly <userlib>:"Filter 1D Array__ogtk.vi"("items to filter"=w709, "array"=w731) -> ("filtered item indices"=w734:i32[])  [unwired: 4 in, 1 out]
          n308 = Index Array(array=w734) -> (element=w717:i32)  [unwired: 1 in]
          n309 = Index Array(array=w718, index=w717) -> (element=w710:string)
          n310 = Index Array(array=w720, index=w717) -> (element=w713:string)
          n311 = Index Array(array=w733, index=w717) -> (element=w728:T8)
          n312 = Index Array(array=w732, index=w717) -> (element=w727:T11)
          n313 = Index Array(array=w725, index=w717) -> (element=w722:cluster{"Lower value":sgl, "Upper value":sgl})
          n314 = Search 1D Array(1D array=w714, element=w710) -> (index of element=w715:i32)  [unwired: 1 in]
          n315 = Search 1D Array(1D array=w714, element=w713) -> (index of element=w712:i32)  [unwired: 1 in]
          n316 = Bundle By Name(cluster=w716, "Camera"=w709, "Motor Alias Y"=w715, "Motor Alias X"=w712) -> (w711:T54)
          n317 = Replace Array Subset(array=w730, new element=w728, index=w719) -> (w726:T8[])
          n318 = Replace Array Subset(array=w729, new element=w727, index=w719) -> (w724:T11[])
          n319 = Replace Array Subset(array=w723, new element=w722, index=w719) -> (w721:cluster{"Lower value":sgl, "Upper value":sgl}[])
        }
        n320 = property on="Cameras and motors" class="Arr (strict)"("Value"=w661) -> ()  [unwired: 2 in, 2 out]
        n321 = Bundle By Name(cluster=w647, "Detection.detection para"=w672, "move properties"=w671, "Detection.thresholds"=w665) -> (w670:T35)
      }
      frame "MotorRefs" {
        n322 = call <vilib>:"Add State(s) to Queue__jki_lib_state_machine.vi"("State(s) in (\"\")"=w739) -> ("States Out"=w738:string)  [unwired: 14 in]
      }
      frame "SetCameraNameControls" {
        # "Initialize the User Interface, here.\n(this is called automatically, by the Macro: Init)"
        n323 = local read "CCDs"() -> (w753:string[])
        n324 = Index Array(array=w753) -> (element #1=w752:string, element #2=w751:string, element #3=w750:string, element #4=w749:string, element #5=w748:string, element #6=w747:string, element #7=w746:string, element #8=w745:string, element #9=w744:string, element #10=w743:string, element #11=w742:string, element #12=w741:string)  [unwired: 12 in]
        n325 = property on="GUIdevice 1" class="Str"("Val(Sgnl)"=w752) -> ()  [unwired: 2 in, 2 out]
        n326 = property on="GUIdevice 2" class="Str"("Val(Sgnl)"=w751) -> ()  [unwired: 2 in, 2 out]
        n327 = property on="GUIdevice 3" class="Str"("Val(Sgnl)"=w750) -> ()  [unwired: 2 in, 2 out]
        n328 = property on="GUIdevice 4" class="Str"("Val(Sgnl)"=w749) -> ()  [unwired: 2 in, 2 out]
        n329 = property on="GUIdevice 5" class="Str"("Val(Sgnl)"=w748) -> ()  [unwired: 2 in, 2 out]
        n330 = property on="GUIdevice 6" class="Str"("Val(Sgnl)"=w747) -> ()  [unwired: 2 in, 2 out]
        n331 = property on="GUIdevice 7" class="Str"("Val(Sgnl)"=w746) -> ()  [unwired: 2 in, 2 out]
        n332 = property on="GUIdevice 8" class="Str"("Val(Sgnl)"=w745) -> ()  [unwired: 2 in, 2 out]
        n333 = property on="GUIdevice 9" class="Str"("Val(Sgnl)"=w744) -> ()  [unwired: 2 in, 2 out]
        n334 = property on="GUIdevice 10" class="Str"("Val(Sgnl)"=w743) -> ()  [unwired: 2 in, 2 out]
        n335 = property on="GUIdevice 11" class="Str"("Val(Sgnl)"=w742) -> ()  [unwired: 2 in, 2 out]
        n336 = property on="GUIdevice 12" class="Str"("Val(Sgnl)"=w741) -> ()  [unwired: 2 in, 2 out]
        n337 = call <vilib>:"Add State(s) to Queue__jki_lib_state_machine.vi"("State(s) in (\"\")"=w757) -> ("States Out"=w756:string)  [unwired: 14 in]
      }
      frame "CameraRefs" {
        w759 = T55 0 items=["Grayscale (U8)", "Grayscale (I16)", "Grayscale (SGL)", "Complex (CSG)", "RGB (U32)", "HSL (U32)", "RGB (U64)", "Grayscale (U16)"] ("Image Type")
        n338 = property on="image::5" class="ImageControl"("Caption.Text"="GUIdevice 5") -> ()  [unwired: 2 in, 2 out]
        n339 = property on="image::7" class="ImageControl"("Caption.Text"="GUIdevice 7") -> ()  [unwired: 2 in, 2 out]
        n340 = property on="image::6" class="ImageControl"("Caption.Text"="GUIdevice 6") -> ()  [unwired: 2 in, 2 out]
        n341 = property on="image::9" class="ImageControl"("Caption.Text"="GUIdevice 9") -> ()  [unwired: 2 in, 2 out]
        n342 = property on="image::1" class="ImageControl"("Caption.Text"="GUIdevice 1") -> ()  [unwired: 2 in, 2 out]
        n343 = property on="image::10" class="ImageControl"("Caption.Text"="GUIdevice 10") -> ()  [unwired: 2 in, 2 out]
        n344 = property on="image::8" class="ImageControl"("Caption.Text"="GUIdevice 8") -> ()  [unwired: 2 in, 2 out]
        n345 = property on="image::2" class="ImageControl"("Caption.Text"="GUIdevice 2") -> ()  [unwired: 2 in, 2 out]
        n346 = property on="image::4" class="ImageControl"("Caption.Text"="GUIdevice 4") -> ()  [unwired: 2 in, 2 out]
        n347 = property on="image::3" class="ImageControl"("Caption.Text"="GUIdevice 3") -> ()  [unwired: 2 in, 2 out]
        n348 = property on="image::11" class="ImageControl"("Caption.Text"="GUIdevice 11") -> ()  [unwired: 2 in, 2 out]
        n349 = property on="image::12" class="ImageControl"("Caption.Text"="GUIdevice 12") -> ()  [unwired: 2 in, 2 out]
        n350 = call "IMAQ Create"("Image Name"="GUIdevice 8", "Image Type"=w759) -> ("New Image"=→"image::8":T5)  [unwired: 3 in, 1 out]
        n351 = call "IMAQ Create"("Image Name"="GUIdevice 9", "Image Type"=w759) -> ("New Image"=→"image::9":T5)  [unwired: 3 in, 1 out]
        n352 = call "IMAQ Create"("Image Name"="GUIdevice 10", "Image Type"=w759) -> ("New Image"=→"image::10":T5)  [unwired: 3 in, 1 out]
        n353 = call "IMAQ Create"("Image Name"="GUIdevice 6", "Image Type"=w759) -> ("New Image"=→"image::6":T5)  [unwired: 3 in, 1 out]
        n354 = call "IMAQ Create"("Image Name"="GUIdevice 7", "Image Type"=w759) -> ("New Image"=→"image::7":T5)  [unwired: 3 in, 1 out]
        n355 = call "IMAQ Create"("Image Name"="GUIdevice 11", "Image Type"=w759) -> ("New Image"=→"image::11":T5)  [unwired: 3 in, 1 out]
        n356 = call "IMAQ Create"("Image Name"="GUIdevice 12", "Image Type"=w759) -> ("New Image"=→"image::12":T5)  [unwired: 3 in, 1 out]
        n357 = call "IMAQ Create"("Image Name"="GUIdevice 2") -> ("New Image"=→"image::2":T5)  [unwired: 4 in, 1 out]
        n358 = call "IMAQ Create"("Image Name"="GUIdevice 4", "Image Type"=w759) -> ("New Image"=→"image::4":T5)  [unwired: 3 in, 1 out]
        n359 = call "IMAQ Create"("Image Name"="GUIdevice 1", "Image Type"=w759) -> ("New Image"=→"image::1":T5)  [unwired: 3 in, 1 out]
        n360 = call "IMAQ Create"("Image Name"="GUIdevice 3", "Image Type"=w759) -> ("New Image"=→"image::3":T5)  [unwired: 3 in, 1 out]
        n361 = call "IMAQ Create"("Image Name"="GUIdevice 5", "Image Type"=w759) -> ("New Image"=→"image::5":T5)  [unwired: 3 in, 1 out]
        n362 = call <vilib>:"Add State(s) to Queue__jki_lib_state_machine.vi"("State(s) in (\"\")"=w787) -> ("States Out"=w786:string)  [unwired: 14 in]
      }
      frame "StartSuperGUI" {
        # "create stop queue for supergui and its clones"
        # "can make an icon"
        # "x100 abort will be dependent on caller VI\nx80 abort will be independent of caller vi, this will abort vi when labview is closed."
        # "Initialize the User Interface, here.\n(this is called automatically, by the Macro: Init)"
        n363 = vi-ref "GUI_Master_subvi_reentrant_queues.vi"() -> (w796:refnum<vi>)
        n364 = call "supergui create stop queue.vi"() -> ("STOP Queue out"=w797:refnum<queue>)  [unwired: 11 in]
        n365 = control-ref of="This Application"() -> (w800:refnum<vi>)
        n366 = property class="VI"(reference=w796) -> ("Path"=w795:path)  [unwired: 1 in, 2 out]
        n367 = control-ref of="This VI"() -> (w799:refnum<vi>)
        n368 = Create User Event(user event datatype=T28 {"EventEnum"=enum."new data", "Device name"="Device name"} ("New Event"), error in=w791) -> (user event=w801:refnum<user-event>, error out=w802:errorcluster)
        "tcp data event 2" <- w801
        n369 = Current VI's Menubar() -> (w798:refnum<k9>)
        n370 = register-events(w801) -> ()  [unwired: 2 in, 2 out]
        n371 = Open VI Reference(type specifier VI Refnum (for type only)=refnum<vi> refnum, vi path=w795, options=256, error in (no error)=w791) -> (vi reference=w806:refnum<vi>, error out=w805:errorcluster)  [unwired: 2 in]
        n372 = call <vilib>:"Add State(s) to Queue__jki_lib_state_machine.vi"("State(s) in (\"\")"=w808) -> ("States Out"=w807:string)  [unwired: 14 in]
        n373 = call-by-ref "Start Asynchronous Call"(reference=w806, error in=w805, "STOP Queue in"=w797, "This Application"=w800, 8:"error in (no error)"=w802, "tcp data event"=w801, "Caller menu reference"=w798, "Caller VI ref"=w799) -> (reference out=w794:refnum<vi>, error out=w790:errorcluster)  [unwired: 5 in, 1 out]
        n374 = Bundle By Name(cluster=w793, "Supergui.SuperGUI ref"=w794, "Supergui.STOP queue"=w797) -> (w792:T35)
      }
      frame "Device Ini" {
        n375 = Empty String/Path?(string/path=w814) -> (empty?=w831:bool)
        n376 = case shown="False" w831 {
          tunnel: w814 -> [w892 _]
          tunnel: [w891 0] -> w830
          frame False {
            n377 = Decimal String To Number(string=w892) -> (number=w891:i32)  [unwired: 2 in, 1 out]
          }
          frame True {
          }
        }
        n378 = flat-sequence {
          tunnel: w835 -> [w838]
          tunnel: [w838] -> w809
          tunnel: w830 -> [w837]
          tunnel: w809 -> [w843]
          tunnel: [w841] -> w817
          frame #0 {
            # "check"
            n379 = Wait (ms)(milliseconds to wait=w837) -> ()  [unwired: 1 out]
          }
          frame #1 {
            # "check if cam images are new"
            n380 = local read "cam means"() -> (w839:sgl[])
            n381 = for {
              tunnel: w843 -> [w846] mode=indexing
              shift-right: [w851] -> w841
              shift-left: string[] [] -> [w852]
              tunnel: [w845] -> w840 mode=indexing
              shift-right: [w849] -> _
              shift-left: w839 -> [w849]
              i -> [w850]
              n382 = call "IMAQ Histograph"("Image"=w846) -> ("error out"=w844:errorcluster, "Mean Value"=w845:sgl)  [unwired: 7 in, 2 out]
              n383 = Index Array(array=w849, index=w850) -> (element=w848:sgl)
              n384 = call <vilib>:"Clear Errors.vi"("error in (no error)"=w844) -> ()  [unwired: 5 in, 2 out]
              n385 = Equal?(x=w845, y=w848) -> (x = y?=w847:bool)
              n386 = case shown="False" w847 {
                tunnel: w852 -> [w855 w856]
                tunnel: [w854 w856] -> w851
                tunnel: w846 -> [w853 _]
                frame False {
                  n387 = Build Array (concatenate)(w855, w853) -> (w854:string[])
                }
                frame True {
                }
              }
            }
            "cam means" <- w840
          }
        }
        n388 = Unbundle By Name(w829) -> ("active cams"=w822:string[])
        n389 = Equal?(x=w814, y="T") -> (x = y?=w812:bool)
        n390 = Equal?(x=w822, y=w817) -> (x = y?=w828:bool[])
        n391 = Empty Array?(array=w822) -> (empty?=w827:bool)
        n392 = Not(x=w827) -> (.not. x?=w826:bool)
        n393 = Build Array (concatenate)(w828, w826) -> (w825:bool[])
        n394 = Array Size(array=w817) -> (size(s)=w821:i32)
        n395 = Array Size(array=w822) -> (size(s)=w820:i32)
        n396 = And Array Elements(Boolean array=w825) -> (logical AND=w818:bool)
        n397 = Equal?(x=w821, y=w820) -> (x = y?=w819:bool)
        n398 = And(x=w819, y=w818) -> (x .and. y?=w816:bool)
        n399 = Not(x=w816) -> (.not. x?=w813:bool)
        n400 = Or(x=w813, y=w812) -> (x .or. y?=w811:bool)
        n401 = call <vilib>:"Add State(s) to Queue__jki_lib_state_machine.vi"("State(s) in (\"\")"=w836) -> ("States Out"=w824:string)  [unwired: 14 in]
        n402 = case shown="True" w811 {
          tunnel: [w859 w874] -> w834
          tunnel: w833 -> [w858 w873]
          tunnel: [w858 w873] -> w832
          tunnel: w829 -> [w859 w870]
          tunnel: w817 -> [_ w863]
          tunnel: w824 -> [w857 w861]
          tunnel: [w857 w866] -> w823
          frame False {
          }
          frame True {
            # "#todo check repercussion of not loading config here"
            # "# active cams changed, perform configuration"
            n403 = local write "#imgs avd so far"(0.0 ("Numeric")) -> ()
            n404 = property on="active CCDs" class="LstBox (strict)"("Item Names"=w863) -> ()  [unwired: 2 in, 2 out]
            n405 = Bundle By Name(cluster=w870, "active cams"=w863) -> (w862:T35)
            n406 = Array Size(array=w863) -> (size(s)=w880:i32)
            n407 = Initialize Array(0.0 ("element"), w880, 0 ("dimension size")) -> (w875:dbl[][])
            n408 = Unbundle By Name(w862) -> ("Detection.img to avg"=w869:i32)
            n409 = Initialize Array(0.0 ("element"), 12 ("dimension size"), w869) -> (w868:dbl[][])
            n410 = for {
              N: 1 -> [_]
              shift-right: [w885] -> w878
              shift-left: timestamp[][] [] ("Time") -> [w887]
              n411 = for {
                N: 12 -> [_]
                tunnel: w887 -> [w890] mode=indexing
                tunnel: [w888] -> w885 mode=indexing
                n412 = Get Date/Time In Seconds() -> (seconds since 1Jan1904=w889:timestamp)
                n413 = Build Array (concatenate)(w890, w889) -> (w888:timestamp[])
              }
            }
            n414 = Bundle By Name(cluster=w862, "Offset X stats"=w875, "Offset Y stats"=w875, "Detection.Centroid X"=w868, "Detection.Centroid Y"=w868, "Mean Centroid X"=w875, "Mean Centroid Y"=w875, "Offset X"=w875, "Offset Y"=w875, "Detection.Size"=w868, "Mean Size"=w875, "Motor X"=w875, "Motor Y"=w875) -> (w874:T35)
            n415 = disable-structure shown="Disabled" {
              disable-tunnel: [w882 _] -> w865
              frame Disabled {
                n416 = property on="config path" class="Str"() -> ("Value"=w883:string)  [unwired: 2 in, 2 out]
                n417 = call <vilib>:"Build State String with Arguments__jki_lib_state_machine.vi"("Arguments (\"\")"=w883, "State"="Load Config" ("State(s) in Front (\"\")")) -> ("State with Arguments"=w882:string)  [unwired: 4 in]
              }
              frame Enabled {
              }
            }
            n418 = property on="Time" class="Arr (strict)"("Value"=w878) -> ()  [unwired: 2 in, 2 out]
            n419 = call <vilib>:"Add State(s) to Queue__jki_lib_state_machine.vi"("State(s) in (\"\")"=w861, "State(s) at Back (\"\")"="active\nCenter" ("State(s) in Front (\"\")")) -> ("States Out"=w867:string)  [unwired: 13 in]
            n420 = call <vilib>:"Add State(s) to Queue__jki_lib_state_machine.vi"("State(s) in (\"\")"=w867, "State(s) at Back (\"\")"=w865) -> ("States Out"=w866:string)  [unwired: 13 in]
            "name array" <- w863
          }
        }
      }
      frame "Save Config" {
        w906 = T27 {"Camera names"=[], "Motor aliases x"=[], "Motor aliases y"=[], "detection para"=[], "thresholds"=[], "move properties"=[], "tdms root"=path "c:/BP_DATAsd"}  # BP Configuration
        n421 = property on="Save Config" class="Bool (strict)"("Value"=FALSE ("Save Config")) -> ()  [unwired: 2 in, 2 out]
        n422 = local read "Cameras and motors"() -> (w901:T4)
        n423 = property on="Motor Alias X" class="Ring (strict)"() -> ("Strings []"=w902:string[])  [unwired: 2 in, 2 out]
        n424 = call "File Dialog"("pattern (all files)"="*.cfg", "pattern label"="config") -> ("selected path"=w896:path)  [unwired: 10 in, 3 out]
        n425 = for {
          tunnel: [w923] -> w905 mode=indexing
          tunnel: [w919] -> w904 mode=indexing
          tunnel: w902 -> [w921]
          tunnel: w901 -> [w924] mode=indexing
          tunnel: [w918] -> w899 mode=indexing
          n426 = Unbundle By Name(w924) -> ("Camera"=w918:string, "Motor Alias X"=w922:u16, "Motor Alias Y"=w920:u16)
          n427 = Index Array(array=w921, index=w920) -> (element=w919:string)
          n428 = Index Array(array=w921, index=w922) -> (element=w923:string)
        }
        n429 = Unbundle By Name(w915) -> ("move properties"=w909:T11[], "Detection.detection para"=w908:T8[], "Detection.thresholds"=w907:cluster{"Lower value":sgl, "Upper value":sgl}[])
        n430 = local read "tdms root"() -> (w898:path)
        n431 = Bundle By Name(cluster=w906, "Camera names"=w899, "move properties"=w909, "detection para"=w908, "thresholds"=w907, "Motor aliases x"=w905, "Motor aliases y"=w904, "tdms root"=w898) -> (w903:T27)
        n432 = disable-structure shown="Enabled" {
          disable-tunnel: w914 -> [w928 w936]
          disable-tunnel: [w927 w935] -> w913
          disable-tunnel: w896 -> [w926 w934]
          disable-tunnel: w903 -> [w925 w937]
          frame Disabled {
            n433 = Open/Create/Replace File(file path (use dialog)=w926, error in=w928, operation (0:open)=T29."replace or create with confirmation") -> (refnum out=w930:refnum<file>, error out=w931:errorcluster)  [unwired: 3 in, 1 out]
            n434 = Write to Binary File(file (use dialog)=w930, data=w925, error in=w931) -> (refnum out=w933:refnum<file>, error out=w932:errorcluster)  [unwired: 3 in, 1 out]
            n435 = Close File(refnum=w933, error in=w932) -> (error out=w927:errorcluster)  [unwired: 1 out]
          }
          frame Enabled {
            n436 = call <userlib>:"MGI Write Anything.vi"("Error In"=w936, "Anything"=w937, "Path (dialog)"=w934) -> ("Error Out"=w935:errorcluster)  [unwired: 6 in, 2 out]
          }
        }
        n437 = Path To String(path=w896) -> (string=w895:string)
        n438 = call <vilib>:"Build State String with Arguments__jki_lib_state_machine.vi"("Arguments (\"\")"=w895, "State"="Load Config" ("State(s) at Back (\"\")")) -> ("State with Arguments"=w894:string)  [unwired: 4 in]
        n439 = call <vilib>:"Add State(s) to Queue__jki_lib_state_machine.vi"("State(s) in Front (\"\")"=w894, "State(s) in (\"\")"=w917) -> ("States Out"=w916:string)  [unwired: 13 in]
      }
      frame "active" {
        # "problem. when trying to change move config or beam\ndet para, it kees getting overwritten here"
        n440 = Empty String/Path?(string/path=w954) -> (empty?=w953:bool)
        n441 = Unbundle By Name(w951) -> ("move properties"=w962:T11[], "Detection.detection para"=w958:T8[], "active ccd"=w944:i32, "active cams"=w943:string[])
        n442 = Unbundle By Name(w951) -> ("dev var alias arrays.dev variable alias Motors X"=w948:string[][], "dev var alias arrays.dev variable alias Motors Y"=w946:string[][])
        n443 = call-poly <userlib>:"Filter 1D Array__ogtk.vi"("items to filter"=w954, "array"=w960) -> ("filtered item indices"=w963:i32[])  [unwired: 4 in, 1 out]
        n444 = Index Array(array=w963) -> (element=w952:i32)  [unwired: 1 in]
        n445 = Select(t=w944, s=w953, f=w952) -> (s? t:f=w942:i32)
        n446 = Index Array(array=w962, index=w942) -> (element=w961:T11)
        n447 = Index Array(array=w958, index=w942) -> (element=w957:T8)
        n448 = property on="move config" class="Clust (strict)"(error in=w940, "Value"=w961) -> (error out=w955:errorcluster)  [unwired: 1 in, 1 out]
        n449 = Index Array(array=w943, index=w942) -> (element=→"Active CCD":string)
        n450 = property on="beam detection para" class="Clust (strict)"(error in=w955, "Value"=w957) -> (error out=w939:errorcluster)  [unwired: 1 in, 1 out]
        n451 = disable-structure shown="Enabled" {
          disable-tunnel: w948 -> [w975 w983]
          disable-tunnel: [w973 w982] -> w947
          disable-tunnel: w946 -> [w971 w981]
          disable-tunnel: [w970 w980] -> w945
          disable-tunnel: w942 -> [w969 w979]
          disable-tunnel: w939 -> [w968 w978]
          disable-tunnel: [w966 w976] -> w938
          frame Disabled {
            n452 = call "Beampointing get set motor position.vi"("Active CCD"=w969, "error in (no error)"=w968, "get or set"=enum16{"get", "set"}."get", "dev variable alias Motors X"=w971) -> ("error out"=w967:errorcluster, "Actual Position"=w970:dbl)  [unwired: 6 in]
            n453 = call "Beampointing get set motor position.vi"("Active CCD"=w969, "error in (no error)"=w967, "get or set"=enum16{"get", "set"}."get", "dev variable alias Motors X"=w975) -> ("error out"=w966:errorcluster, "Actual Position"=w973:dbl)  [unwired: 6 in]
          }
          frame Enabled {
            n454 = call "Beampointing get motor position tcp.vi"("Active CCD"=w979, "error in (no error)"=w978, "dev variable alias Motors X"=w981) -> ("error out"=w977:errorcluster, "value"=w980:dbl)  [unwired: 7 in]
            n455 = call "Beampointing get motor position tcp.vi"("Active CCD"=w979, "error in (no error)"=w977, "dev variable alias Motors X"=w983) -> ("error out"=w976:errorcluster, "value"=w982:dbl)  [unwired: 7 in]
          }
        }
        n456 = call <vilib>:"Add State(s) to Queue__jki_lib_state_machine.vi"("State(s) in (\"\")"=w965) -> ("States Out"=w964:string)  [unwired: 14 in]
        n457 = Bundle By Name(cluster=w951, "active ccd"=w942) -> (w959:T35)
        n458 = property on="Position 1" class="DigNum (strict)"(error in=w938, "Value"=w947) -> (error out=w950:errorcluster)  [unwired: 1 in, 1 out]
        n459 = property on="Position 2" class="DigNum (strict)"(error in=w950, "Value"=w945) -> (error out=w956:errorcluster)  [unwired: 1 in, 1 out]
      }
      frame "set detection params from control" {
        # "Your code here.\n(You can make a copy of, or modify, this frame)"
        n460 = Unbundle By Name(w989) -> ("Detection.detection para"=w985:T8[], "active ccd"=w990:i32)
        n461 = Replace Array Subset(array=w985, new element="beam detection para", index=w990) -> (w986:T8[])
        n462 = Bundle By Name(cluster=w989, "Detection.detection para"=w986) -> (w988:T35)
        n463 = call <vilib>:"Add State(s) to Queue__jki_lib_state_machine.vi"("State(s) in (\"\")"=w993) -> ("States Out"=w992:string)  [unwired: 14 in]
      }
      frame "Motor Config" {
        n464 = for {
          tunnel: w1002 -> [w1024]
          tunnel: "Cameras and motors" -> [w1023] mode=indexing
          tunnel: [w1011] -> w1000 mode=indexing
          tunnel: [w1016] -> w999 mode=indexing
          tunnel: [w1014] -> w997 mode=indexing
          tunnel: [w1012] -> w996 mode=indexing
          tunnel: w995 -> [w1009]
          tunnel: [w1008] -> w994
          n465 = Unbundle By Name(w1024) -> ("dev var alias arrays.dev variable alias"=w1020:string[][])
          n466 = Index Array(array=w1020, index (col)=2 ("disabled index (col)")) -> (element=w1019:string[])  [unwired: 1 in]
          n467 = Unbundle By Name(w1023) -> ("Motor Alias X"=w1028:u16, "Motor Alias Y"=w1018:u16)
          n468 = property on="Motor Alias X" class="Ring (strict)"() -> ("Strings []"=w1017:string[])  [unwired: 2 in, 2 out]
          n469 = Index Array(array=w1017, index=w1028) -> (element=w1027:string)
          n470 = Search 1D Array(1D array=w1019, element=w1027) -> (index of element=w1026:i32)  [unwired: 1 in]
          n471 = Index Array(array=w1020, index (row)=w1026) -> (element=w1011:string[])  [unwired: 1 in]
          n472 = Index Array(array=w1017, index=w1018) -> (element=w1021:string)
          n473 = Search 1D Array(1D array=w1019, element=w1021) -> (index of element=w1022:i32)  [unwired: 1 in]
          n474 = Index Array(array=w1020, index (row)=w1022) -> (element=w1016:string[])  [unwired: 1 in]
          n475 = call "get set udp value from dev var alias array.vi"("slow timeout ms (3000)"=1000, "error in (no error)"=w1009, "get or set"=enum16{"get", "set"}."get", "dev variable alias Motors X"=w1016) -> ("error out"=w1010:errorcluster, "Numeric"=w1014:dbl)  [unwired: 6 in]
          n476 = call "get set udp value from dev var alias array.vi"("slow timeout ms (3000)"=1000, "error in (no error)"=w1010, "get or set"=enum16{"get", "set"}."get", "dev variable alias Motors X"=w1011) -> ("error out"=w1008:errorcluster, "Numeric"=w1012:dbl)  [unwired: 6 in]
        }
        n477 = call <vilib>:"Add State(s) to Queue__jki_lib_state_machine.vi"("State(s) in (\"\")"=w1005) -> ("States Out"=w1004:string)  [unwired: 14 in]
        n478 = Bundle By Name(cluster=w1002, "dev var alias arrays.dev variable alias Motors X"=w1000, "dev var alias arrays.dev variable alias Motors Y"=w999, "Motor positions.Positions x"=w996, "Motor positions.Positions y"=w997) -> (w1003:T35)
      }
      frame "set move props from control" {
        # "Your code here.\n(You can make a copy of, or modify, this frame)"
        n479 = Unbundle By Name(w1031) -> ("move properties"=w1035:T11[], "active ccd"=w1034:i32)
        n480 = Replace Array Subset(array=w1035, new element="move config", index=w1034) -> (w1032:T11[])
        n481 = Bundle By Name(cluster=w1031, "move properties"=w1032) -> (w1030:T35)
        n482 = call <vilib>:"Add State(s) to Queue__jki_lib_state_machine.vi"("State(s) in (\"\")"=w1038) -> ("States Out"=w1037:string)  [unwired: 14 in]
      }
      frame "set thresholds" {
        # "Your code here.\n(You can make a copy of, or modify, this frame)"
        n483 = Unbundle By Name(w1042) -> ("Detection.thresholds"=w1045:cluster{"Lower value":sgl, "Upper value":sgl}[], "active ccd"=w1044:i32)
        n484 = Replace Array Subset(array=w1045, new element="thresholds", index=w1044) -> (w1043:cluster{"Lower value":sgl, "Upper value":sgl}[])
        n485 = Bundle By Name(cluster=w1042, "Detection.thresholds"=w1043) -> (w1041:T35)
        n486 = call <vilib>:"Add State(s) to Queue__jki_lib_state_machine.vi"("State(s) in (\"\")"=w1048) -> ("States Out"=w1047:string)  [unwired: 14 in]
      }
      frame "----------Centroid & Move----------" {
        # "Template Separator\n(You can make a copy of, or modify, this frame)"
        n487 = call <vilib>:"Add State(s) to Queue__jki_lib_state_machine.vi"("State(s) in (\"\")"=w1053) -> ("States Out"=w1052:string)  [unwired: 14 in]
      }
      frame "detected" {
        n488 = Unbundle By Name(w1064) -> ("Offset X"=w1096:dbl[][], "Offset Y"=w1095:dbl[][], "Detection.Size"=w1094:dbl[][], "Mean Size"=w1093:dbl[][], "Time"=w1090:timestamp[][], "Motor X"=w1073:dbl[][], "Motor positions"=w1072:T36, "Motor Y"=w1071:dbl[][])  [unwired: 1 out]
        n489 = Spreadsheet String To Array(format string="%s", spreadsheet string=w1076, array type (2D Dbl)=string[] []) -> (array=w1067:string[])  [unwired: 1 in]
        n490 = for {
          tunnel: w1068 -> [w1108] mode=indexing
          tunnel: w1067 -> [w1107]
          tunnel: [w1106] -> w1066 mode=indexing
          n491 = for {
            tunnel: w1108 -> [w1111]
            tunnel: [w1110] -> w1105 mode=indexing
            tunnel: w1107 -> [w1109] mode=indexing
            n492 = Equal?(x=w1111, y=w1109) -> (x = y?=w1110:bool)
          }
          n493 = Or Array Elements(Boolean array=w1105) -> (logical OR=w1106:bool)
        }
        n494 = local read "Cameras and motors"() -> (w1054:T4)
        n495 = Unbundle By Name(w1064) -> ("Mean Centroid X"=w1099:dbl[][], "Mean Centroid Y"=w1098:dbl[][], "Detection.Centroid X"=w1101:dbl[][], "Detection.Centroid Y"=w1100:dbl[][])
        n496 = call <vilib>:"Add State(s) to Queue__jki_lib_state_machine.vi"("State(s) in (\"\")"=w1075) -> ("States Out"=w1074:string)  [unwired: 14 in]
        n497 = for {
          tunnel: w1101 -> [w1161]
          tunnel: w1100 -> [w1160]
          tunnel: w1099 -> [w1159]
          tunnel: w1098 -> [w1158]
          tunnel: [w1157] -> w1087 mode=indexing
          tunnel: [w1156] -> w1097 mode=indexing
          tunnel: w1096 -> [w1155]
          tunnel: w1095 -> [w1154]
          tunnel: [w1153] -> w1065 mode=indexing
          tunnel: [w1152] -> w1088 mode=indexing
          tunnel: w1094 -> [w1151]
          tunnel: w1093 -> [w1150]
          tunnel: [w1149] -> w1092 mode=indexing
          tunnel: w1090 -> [w1148]
          tunnel: [w1147] -> w1089 mode=indexing
          tunnel: w1073 -> [w1144]
          tunnel: w1072 -> [w1117]
          tunnel: w1071 -> [w1143]
          tunnel: [w1123] -> w1070 mode=indexing
          tunnel: [w1122] -> w1069 mode=indexing
          tunnel: w1066 -> [w1121]
          tunnel: w1055 -> [w1119]
          tunnel: w1054 -> [_] mode=indexing
          i -> [w1113]
          n498 = Index Array(array=w1119, index=w1113) -> (element=w1118:T20)
          n499 = Unbundle By Name(w1117) -> ("Positions x"=w1116:dbl[], "Positions y"=w1114:dbl[])
          n500 = Unbundle By Name(w1118) -> ("Target.X::12"=w1127:refnum<vi>, "Target.Y::12"=w1126:refnum<vi>)
          n501 = Index Array(array=w1144, index (row)=w1113) -> (element=w1145:dbl[])  [unwired: 1 in]
          n502 = Index Array(array=w1116, index=w1113) -> (element=w1115:dbl)
          n503 = Index Array(array=w1143, index (row)=w1113) -> (element=w1146:dbl[])  [unwired: 1 in]
          n504 = Index Array(array=w1121, index=w1113) -> (element=w1120:bool)
          n505 = Index Array(array=w1159, index (row)=w1113) -> (element=w1139:dbl[])  [unwired: 1 in]
          n506 = Index Array(array=w1158, index (row)=w1113) -> (element=w1140:dbl[])  [unwired: 1 in]
          n507 = Index Array(array=w1161, index (row)=w1113) -> (element=w1142:dbl[])  [unwired: 1 in]
          n508 = Index Array(array=w1160, index (row)=w1113) -> (element=w1141:dbl[])  [unwired: 1 in]
          n509 = Index Array(array=w1155, index (row)=w1113) -> (element=w1135:dbl[])  [unwired: 1 in]
          n510 = Index Array(array=w1154, index (row)=w1113) -> (element=w1134:dbl[])  [unwired: 1 in]
          n511 = Index Array(array=w1151, index (row)=w1113) -> (element=w1132:dbl[])  [unwired: 1 in]
          n512 = Index Array(array=w1150, index (row)=w1113) -> (element=w1131:dbl[])  [unwired: 1 in]
          n513 = Index Array(array=w1148, index (row)=w1113) -> (element=w1128:timestamp[])  [unwired: 1 in]
          n514 = Index Array(array=w1114, index=w1113) -> (element=w1112:dbl)
          n515 = property class="DigNum (strict)"(reference=w1127) -> ("Value"=w1125:dbl)  [unwired: 1 in, 2 out]
          n516 = property class="DigNum (strict)"(reference=w1126) -> ("Value"=w1124:dbl)  [unwired: 1 in, 2 out]
          n517 = call <vilib>:"Std Deviation and Variance.vi"("X"=w1142) -> ("mean"=w1138:dbl)  [unwired: 1 in, 2 out]
          n518 = call <vilib>:"Std Deviation and Variance.vi"("X"=w1141) -> ("mean"=w1137:dbl)  [unwired: 1 in, 2 out]
          n519 = call <vilib>:"Std Deviation and Variance.vi"("X"=w1132) -> ("mean"=w1130:dbl)  [unwired: 1 in, 2 out]
          n520 = Get Date/Time In Seconds() -> (seconds since 1Jan1904=w1129:timestamp)
          n521 = Subtract(x=w1125, y=w1138) -> (x-y=w1136:dbl)
          n522 = Subtract(x=w1124, y=w1137) -> (x-y=w1133:dbl)
          n523 = case shown="True" w1120 {
            tunnel: [w1174 w1193] -> w1157
            tunnel: [w1162 w1192] -> w1156
            tunnel: [w1163 w1191] -> w1153
            tunnel: [w1164 w1190] -> w1152
            tunnel: [w1165 w1189] -> w1149
            tunnel: [w1166 w1188] -> w1147
            tunnel: w1140 -> [w1172 w1187]
            tunnel: w1139 -> [w1173 w1186]
            tunnel: w1138 -> [_ w1185]
            tunnel: w1137 -> [_ w1184]
            tunnel: w1136 -> [_ w1183]
            tunnel: w1135 -> [w1171 w1182]
            tunnel: w1134 -> [w1170 w1181]
            tunnel: w1133 -> [_ w1180]
            tunnel: w1131 -> [w1169 w1179]
            tunnel: w1130 -> [_ w1178]
            tunnel: w1129 -> [w1167 w1177]
            tunnel: w1128 -> [w1168 w1176]
            frame False {
              w1175 = 0.0
              n524 = Build Array (concatenate)(w1173, w1175) -> (w1174:dbl[])
              n525 = Build Array (concatenate)(w1172, w1175) -> (w1162:dbl[])
              n526 = Build Array (concatenate)(w1171, w1175) -> (w1163:dbl[])
              n527 = Build Array (concatenate)(w1170, w1175) -> (w1164:dbl[])
              n528 = Build Array (concatenate)(w1169, w1175) -> (w1165:dbl[])
              n529 = Build Array (concatenate)(w1168, w1167) -> (w1166:timestamp[])
            }
            frame True {
              n530 = Build Array (concatenate)(w1186, w1185) -> (w1193:dbl[])
              n531 = Build Array (concatenate)(w1187, w1184) -> (w1192:dbl[])
              n532 = Build Array (concatenate)(w1182, w1183) -> (w1191:dbl[])
              n533 = Build Array (concatenate)(w1181, w1180) -> (w1190:dbl[])
              n534 = Build Array (concatenate)(w1179, w1178) -> (w1189:dbl[])
              n535 = Build Array (concatenate)(w1176, w1177) -> (w1188:timestamp[])
            }
          }
          n536 = Build Array (concatenate)(w1145, w1115) -> (w1123:dbl[])
          n537 = Build Array (concatenate)(w1146, w1112) -> (w1122:dbl[])
        }
        n538 = local write "#imgs avd so far"(0.0 ("Numeric")) -> ()
        n539 = Array Size(array=w1065) -> (size(s)=w1086:i32[])
        n540 = Index Array(array=w1086, index=1) -> (element=w1084:i32)
        "History Index" <- w1084
        n541 = call <vilib>:"Add State(s) to Queue__jki_lib_state_machine.vi"("State(s) in (\"\")"=w1074, "State(s) at Back (\"\")"="Check Move\ntdms" ("State(s) at Back (\"\")")) -> ("States Out"=w1078:string)  [unwired: 13 in]
        n542 = Unbundle By Name(w1064) -> ("Detection.img to avg"=w1061:i32)
        n543 = Initialize Array(0.0 ("element"), 12 ("dimension size"), w1061) -> (w1060:dbl[][])
        n544 = Bundle By Name(cluster=w1064, "Detection.Centroid X"=w1060, "Detection.Centroid Y"=w1060, "Mean Centroid X"=w1087, "Mean Centroid Y"=w1097, "Offset X"=w1065, "Offset Y"=w1088, "Mean Size"=w1092, "Detection.Size"=w1060, "Time"=w1089, "Motor X"=w1070, "Motor Y"=w1069) -> (w1057:T35)
        n545 = Greater?(x=w1084, y="History Size") -> (0:w1082:bool)
        n546 = Select(t="history" ("State(s) at Back (\"\")"), s=w1082, f="") -> (s? t:f=w1079:string)
        n547 = call <vilib>:"Add State(s) to Queue__jki_lib_state_machine.vi"("State(s) in (\"\")"=w1078, "State(s) at Back (\"\")"=w1079) -> ("States Out"=w1059:string)  [unwired: 13 in]
        n548 = call <vilib>:"Add State(s) to Queue__jki_lib_state_machine.vi"("State(s) in (\"\")"=w1059) -> ("States Out"=w1058:string)  [unwired: 14 in]
      }
      frame "Check Move" {
        n549 = Unbundle By Name(w1204) -> ("move properties"=w1214:T11[], "Mean Size"=w1213:dbl[][], "move properties"=w1212:T11[], "Offset X"=w1211:dbl[][], "Offset Y"=w1210:dbl[][], "active cams"=w1209:string[])
        n550 = Unbundle By Name(w1204) -> ("steps speed X"=w1203:dbl[], "steps speed Y"=w1202:dbl[])
        n551 = for {
          tunnel: w1212 -> [w1254]
          tunnel: w1211 -> [w1252]
          tunnel: w1210 -> [w1250]
          tunnel: w1213 -> [w1258]
          tunnel: [w1268] -> w1198 mode=indexing
          tunnel: [w1264] -> w1196 mode=indexing
          tunnel: w1209 -> [w1259] mode=indexing
          tunnel: [w1285] -> w1215 mode=indexing
          tunnel: [w1284] -> w1207 mode=indexing
          tunnel: w1214 -> [w1257]
          tunnel: [w1236] -> w1199 mode=indexing
          tunnel: [w1248] -> w1197 mode=indexing
          tunnel: "Speedmode" -> [w1262]
          tunnel: w1206 -> [w1260]
          shift-right: [w1241] -> w1201
          shift-left: w1203 -> [w1246]
          shift-right: [w1240] -> w1200
          shift-left: w1202 -> [w1245]
          tunnel: [w1237] -> w1194 mode=indexing
          n552 = call-poly <userlib>:"Filter 1D Array__ogtk.vi"("items to filter"=w1259, "array"=w1260) -> ("filtered item indices"=w1261:i32[])  [unwired: 4 in, 1 out]
          n553 = Index Array(array=w1261) -> (element=w1244:i32)  [unwired: 1 in]
          n554 = Index Array(array=w1257, index=w1244) -> (element=w1256:T11)
          n555 = Index Array(array=w1258, index (row)=w1244) -> (element=w1255:dbl[])  [unwired: 1 in]
          n556 = Index Array(array=w1254, index=w1244) -> (element=w1253:T11)
          n557 = Index Array(array=w1252, index (row)=w1244) -> (element=w1251:dbl[])  [unwired: 1 in]
          n558 = Index Array(array=w1250, index (row)=w1244) -> (element=w1249:dbl[])  [unwired: 1 in]
          n559 = Unbundle By Name(w1253) -> ("Tolerance [%]"=w1278:dbl)
          n560 = Reverse 1D Array(array=w1251) -> (reversed array=w1283:dbl[])
          n561 = Reverse 1D Array(array=w1249) -> (reversed array=w1282:dbl[])
          n562 = Reverse 1D Array(array=w1255) -> (reversed array=w1277:dbl[])
          n563 = Unbundle By Name(w1256) -> ("Stepsize"=w1239:dbl, "enable feedback"=w1267:bool)
          n564 = Index Array(array=w1283) -> (element=w1281:dbl)  [unwired: 1 in]
          n565 = Index Array(array=w1282) -> (element=w1280:dbl)  [unwired: 1 in]
          n566 = Index Array(array=w1277) -> (element=w1276:dbl)  [unwired: 1 in]
          n567 = Absolute Value(x=w1281) -> (abs(x)=w1247:dbl)
          n568 = Absolute Value(x=w1280) -> (abs(x)=w1263:dbl)
          n569 = Square Root(x=w1276) -> (sqrt(x)=w1275:dbl)
          n570 = Divide(x=w1278, y=100.0) -> (x/y=w1238:dbl)
          n571 = Multiply(x=w1275, y=w1238) -> (x*y=w1237:dbl)
          n572 = Not Equal To 0?(x=w1263) -> (x != 0?=w1265:bool)
          n573 = Not Equal To 0?(x=w1247) -> (x != 0?=w1270:bool)
          n574 = Greater Or Equal?(x=w1247, y=w1237) -> (x >= y?=w1269:bool)
          n575 = Greater Or Equal?(x=w1263, y=w1237) -> (x >= y?=w1266:bool)
          n576 = call "speedmode.vi"("offset X"=w1247, "offset Y"=w1263, "beamsize x tolerance"=w1237, "Speedmode @"=w1262, "step size"=w1239) -> ("steps speed Y"=w1242:dbl, "steps speed X"=w1243:dbl, "speedmode X"=w1236:bool, "speedmode Y"=w1248:bool)  [unwired: 3 in]
          n577 = Compound Arithmetic op=AND(w1267, w1270, w1269) -> (w1268:bool)
          n578 = Compound Arithmetic op=AND(w1267, w1266, w1265) -> (w1264:bool)
          n579 = Boolean To (0,1)(Boolean=w1264) -> (0, 1=w1271:i16)
          n580 = Multiply(x=w1271, y=w1263) -> (x*y=w1272:dbl)
          n581 = Boolean To (0,1)(Boolean=w1268) -> (0, 1=w1274:i16)
          n582 = Replace Array Subset(array=w1246, new element=w1243, index=w1244) -> (w1241:dbl[])
          n583 = Replace Array Subset(array=w1245, new element=w1242, index=w1244) -> (w1240:dbl[])
          n584 = Multiply(x=w1274, y=w1247) -> (x*y=w1273:dbl)
          n585 = Bundle(w1272, "GUIdevice 8"=w1259) -> (w1284:cluster{dbl, "GUIdevice 8":string})  [unwired: 1 in]
          n586 = Bundle(w1273, "GUIdevice 8"=w1259) -> (w1285:cluster{dbl, "GUIdevice 8":string})  [unwired: 1 in]
        }
        "required X" <- w1198
        "required Y" <- w1196
        "tolerances (pix)" <- w1194
        n587 = case shown="False" "Align" {
          tunnel: w1215 -> [w1291 w1296]
          tunnel: w1207 -> [w1290 w1293]
          tunnel: [w1289 w1295] -> w1218
          tunnel: [w1288 w1292] -> w1217
          frame False {
            n588 = Sort 1D Array(array=w1290) -> (sorted array=w1287:cluster{dbl, "GUIdevice 8":string}[])
            n589 = Sort 1D Array(array=w1291) -> (sorted array=w1286:cluster{dbl, "GUIdevice 8":string}[])
            n590 = Reverse 1D Array(array=w1287) -> (reversed array=w1288:cluster{dbl, "GUIdevice 8":string}[])
            n591 = Reverse 1D Array(array=w1286) -> (reversed array=w1289:cluster{dbl, "GUIdevice 8":string}[])
          }
          frame True {
            w1294 = cluster{dbl, "GUIdevice 8":string}[] [] ("Array")
            n592 = for {
              shift-right: [w1306] -> w1295
              shift-left: w1294 -> [w1308]
              tunnel: w1296 -> [w1307] mode=indexing
              n593 = Unbundle(w1307) -> (w1310:dbl)  [unwired: 1 out]
              n594 = Not Equal To 0?(x=w1310) -> (x != 0?=w1309:bool)
              n595 = case shown="True" w1309 {
                tunnel: w1308 -> [w1311 w1314]
                tunnel: w1307 -> [_ w1313]
                tunnel: [w1311 w1312] -> w1306
                frame False {
                }
                frame True {
                  n596 = Build Array (concatenate)(w1314, w1313) -> (w1312:cluster{dbl, "GUIdevice 8":string}[])
                }
              }
            }
            n597 = for {
              shift-right: [w1297] -> w1292
              shift-left: w1294 -> [w1299]
              tunnel: w1293 -> [w1298] mode=indexing
              n598 = Unbundle(w1298) -> (w1301:dbl)  [unwired: 1 out]
              n599 = Not Equal To 0?(x=w1301) -> (x != 0?=w1300:bool)
              n600 = case shown="True" w1300 {
                tunnel: w1299 -> [w1302 w1305]
                tunnel: w1298 -> [_ w1304]
                tunnel: [w1302 w1303] -> w1297
                frame False {
                }
                frame True {
                  n601 = Build Array (concatenate)(w1305, w1304) -> (w1303:cluster{dbl, "GUIdevice 8":string}[])
                }
              }
            }
          }
        }
        n602 = call <vilib>:"Add State(s) to Queue__jki_lib_state_machine.vi"("State(s) in (\"\")"=w1221) -> ("States Out"=w1220:string)  [unwired: 14 in]
        n603 = Bundle By Name(cluster=w1204, "speedmode X"=w1199, "speedmode Y"=w1197, "steps speed X"=w1201, "steps speed Y"=w1200) -> (w1205:T35)
        n604 = Index Array(array=w1217) -> (element=w1222:cluster{dbl, "GUIdevice 8":string})  [unwired: 1 in]
        n605 = Index Array(array=w1218) -> (element=w1223:cluster{dbl, "GUIdevice 8":string})  [unwired: 1 in]
        n606 = Empty Array?(array=w1217) -> (empty?=w1225:bool)
        n607 = Unbundle(w1223) -> (w1231:dbl)  [unwired: 1 out]
        n608 = Unbundle(w1222) -> (w1227:dbl)  [unwired: 1 out]
        n609 = Unbundle By Name(w1205) -> ("Feedback global"=w1232:bool)
        n610 = Empty Array?(array=w1218) -> (empty?=w1229:bool)
        n611 = property on="autodetect" class="Bool (strict)"("Value"=FALSE ("autodetect")) -> ()  [unwired: 2 in, 2 out]
        n612 = Equal To 0?(x=w1231) -> (x = 0?=w1230:bool)
        n613 = Equal To 0?(x=w1227) -> (x = 0?=w1226:bool)
        n614 = Or(x=w1230, y=w1229) -> (x .or. y?=w1228:bool)
        n615 = Or(x=w1226, y=w1225) -> (x .or. y?=w1224:bool)
        n616 = case shown="True" w1232 {
          tunnel: w1228 -> [_ w1333]
          tunnel: w1218 -> [_ w1332]
          tunnel: w1224 -> [_ w1330]
          tunnel: w1217 -> [_ w1329]
          tunnel: w1220 -> [w1315 w1328]
          tunnel: [w1315 w1327] -> w1233
          tunnel: w1199 -> [_ w1326]
          tunnel: w1198 -> [_ w1325]
          tunnel: w1197 -> [_ w1324]
          tunnel: w1196 -> [_ w1323]
          frame False {
          }
          frame True {
            n617 = case shown="False" w1333 {
              tunnel: w1332 -> [w1357 _]
              tunnel: w1328 -> [w1353 w1358]
              tunnel: [w1351 w1358] -> w1331
              frame False {
                n618 = Index Array(array=w1357) -> (element=w1356:cluster{dbl, "GUIdevice 8":string})  [unwired: 1 in]
                n619 = Unbundle By Name(w1356) -> ("GUIdevice 8"=w1355:string)
                n620 = call <vilib>:"Build State String with Arguments__jki_lib_state_machine.vi"("Arguments (\"\")"=w1355, "State"="Move X") -> ("State with Arguments"=w1352:string)  [unwired: 4 in]
                n621 = call <vilib>:"Add State(s) to Queue__jki_lib_state_machine.vi"("State(s) in (\"\")"=w1353, "State(s) at Back (\"\")"=w1352) -> ("States Out"=w1351:string)  [unwired: 13 in]
              }
              frame True {
              }
            }
            n622 = case shown="False" w1330 {
              tunnel: w1329 -> [w1349 _]
              tunnel: w1331 -> [w1345 w1350]
              tunnel: [w1343 w1350] -> w1327
              frame False {
                n623 = Index Array(array=w1349) -> (element=w1348:cluster{dbl, "GUIdevice 8":string})  [unwired: 1 in]
                n624 = Unbundle By Name(w1348) -> ("GUIdevice 8"=w1347:string)
                n625 = call <vilib>:"Build State String with Arguments__jki_lib_state_machine.vi"("Arguments (\"\")"=w1347, "State"="Move Y") -> ("State with Arguments"=w1344:string)  [unwired: 4 in]
                n626 = call <vilib>:"Add State(s) to Queue__jki_lib_state_machine.vi"("State(s) in (\"\")"=w1345, "State(s) at Back (\"\")"=w1344) -> ("States Out"=w1343:string)  [unwired: 13 in]
              }
              frame True {
              }
            }
            n627 = for {
              tunnel: w1326 -> [w1342] mode=indexing
              tunnel: w1325 -> [w1341] mode=indexing
              tunnel: [w1340] -> w1322 mode=indexing
              n628 = And(x=w1342, y=w1341) -> (x .and. y?=w1340:bool)
            }
            n629 = for {
              tunnel: w1324 -> [w1339] mode=indexing
              tunnel: w1323 -> [w1338] mode=indexing
              tunnel: [w1337] -> w1321 mode=indexing
              n630 = And(x=w1339, y=w1338) -> (x .and. y?=w1337:bool)
            }
            n631 = Or Array Elements(Boolean array=w1322) -> (logical OR=w1320:bool)
            n632 = Or Array Elements(Boolean array=w1321) -> (logical OR=w1319:bool)
            n633 = Or(x=w1320, y=w1319) -> (x .or. y?=w1318:bool)
            n634 = property on="alarms" class="Bool (strict)"() -> ("Value"=w1317:bool)  [unwired: 2 in, 2 out]
            n635 = And(x=w1317, y=w1318) -> (x .and. y?=w1316:bool)
            n636 = case shown="True" w1316 {
              frame False {
              }
              frame True {
                n637 = call <vilib>:"Beep.vi"("use system alert? (T)"=FALSE, "duration (msec)"=u32 750, "frequency (Hz)"=u32 750) -> ()  [unwired: 9 in]
              }
            }
          }
        }
        n638 = call <vilib>:"Add State(s) to Queue__jki_lib_state_machine.vi"("State(s) in (\"\")"=w1220, "State(s) at Back (\"\")"=w1233) -> ("States Out"=w1235:string)  [unwired: 13 in]
      }
      frame "Move X" {
        # "Your code here.\n(You can make a copy of, or modify, this frame)"
        n639 = Unbundle By Name(w1372) -> ("Offset X"=w1384:dbl[][])
        n640 = call-poly <userlib>:"Filter 1D Array__ogtk.vi"("items to filter"=w1378, "array"=w1385) -> ("filtered item indices"=w1381:i32[])  [unwired: 4 in, 1 out]
        n641 = Unbundle By Name(w1372) -> ("dev var alias arrays.dev variable alias Motors X"=w1374:string[][])
        n642 = Unbundle By Name(w1372) -> ("move properties"=w1377:T11[])
        n643 = for {
          tunnel: w1381 -> [w1413] mode=indexing
          tunnel: w1377 -> [w1417]
          shift-right: [w1412] -> w1379
          shift-left: i32[] [] ("filtered item indices") -> [w1415]
          n644 = Index Array(array=w1417, index=w1413) -> (element=w1416:T11)
          n645 = Unbundle By Name(w1416) -> ("enable feedback"=w1414:bool)
          n646 = case shown="True" w1414 {
            tunnel: w1415 -> [w1418 w1421]
            tunnel: w1413 -> [_ w1420]
            tunnel: [w1418 w1419] -> w1412
            frame False {
            }
            frame True {
              n647 = Build Array (concatenate)(w1421, w1420) -> (w1419:i32[])
            }
          }
        }
        n648 = Index Array(array=w1379) -> (element=w1369:i32)  [unwired: 1 in]
        n649 = call "Beampointing get set motor position.vi"("Active CCD"=w1369, "error in (no error)"=w1367, "get or set"=enum16{"get", "set"}."get", "dev variable alias Motors X"=w1374) -> ("error out"=w1365:errorcluster, "Actual Position"=w1373:dbl)  [unwired: 6 in]
        n650 = Index Array(array=w1384, index (row)=w1369) -> (element=w1383:dbl[])  [unwired: 1 in]
        n651 = Reverse 1D Array(array=w1383) -> (reversed array=w1382:dbl[])
        n652 = Index Array(array=w1382) -> (element=w1363:dbl)  [unwired: 1 in]
        n653 = Index Array(array=w1377, index=w1369) -> (element=w1359:T11)
        n654 = Unbundle By Name(w1359) -> ("Invert Direction X"=w1364:bool, "enable feedback"=w1366:bool)
        n655 = local read "Align"() -> (w1361:bool)
        n656 = call "relative move from offset and calibration.vi"("Align"=w1361, "axis"=enum16{"x", "y"}."x", "Offset"=w1363, "element"=w1359) -> ("relative move out"=w1362:dbl)  [unwired: 7 in]
        n657 = case shown="No Error" w1365 {
          selector: w1365 -> [w1389 w1410]
          tunnel: w1364 -> [_ _]
          tunnel: w1366 -> [w1399 _]
          tunnel: w1374 -> [w1398 _]
          tunnel: w1373 -> [w1397 _]
          tunnel: w1372 -> [w1396 w1411]
          tunnel: [w1392 w1411] -> w1371
          tunnel: w1369 -> [w1391 _]
          tunnel: w1362 -> [w1390 _]
          tunnel: [w1388 w1410] -> w1368
          frame No Error {
            n658 = case shown="True" w1399 {
              tunnel: w1390 -> [_ w1409]
              tunnel: w1398 -> [_ w1407]
              tunnel: w1391 -> [_ w1406]
              tunnel: w1397 -> [w1400 w1404]
              tunnel: [w1400 w1403] -> w1393
              tunnel: w1389 -> [_ w1402]
              tunnel: [_ w1401] -> w1388
              frame False {
              }
              frame True {
                n659 = Add(x=w1404, y=w1409) -> (x+y=w1405:dbl)
                n660 = call "Beampointing get set motor position.vi"("Active CCD"=w1406, "error in (no error)"=w1402, "Set position"=w1405, "get or set"=enum16{"get", "set"}."set", "dev variable alias Motors X"=w1407) -> ("error out"=w1401:errorcluster, "Actual Position"=w1403:dbl)  [unwired: 5 in]
              }
            }
            n661 = Unbundle By Name(w1396) -> ("Motor positions.Positions x"=w1395:dbl[])
            n662 = Replace Array Subset(array=w1395, new element=w1393, index=w1391) -> (w1394:dbl[])
            n663 = Bundle By Name(cluster=w1396, "Motor positions.Positions x"=w1394) -> (w1392:T35)
          }
          frame Error {
          }
        }
        n664 = call <vilib>:"Build State String with Arguments__jki_lib_state_machine.vi"("Arguments (\"\")"=w1378, "State"="Wait" ("State(s) in Front (\"\")")) -> ()  [unwired: 4 in, 1 out]
        n665 = call <vilib>:"Add State(s) to Queue__jki_lib_state_machine.vi"("State(s) in (\"\")"=w1387) -> ("States Out"=w1386:string)  [unwired: 14 in]
        "Moving X" <- w1378
      }
      frame "ManMove X" {
        # "Your code here.\n(You can make a copy of, or modify, this frame)"
        n666 = Unbundle By Name(w1427) -> ("dev var alias arrays.dev variable alias Motors X"=w1431:string[][])
        n667 = Unbundle By Name(w1427) -> ("move properties"=w1441:T11[], "active ccd"=w1424:i32, "active cams"=w1439:string[])  [unwired: 1 out]
        n668 = Index Array(array=w1439, index=w1424) -> (element=w1437:string)
        n669 = call "Beampointing get set motor position.vi"("Active CCD"=w1424, "get or set"=enum16{"get", "set"}."get", "dev variable alias Motors X"=w1431) -> ("error out"=w1422:errorcluster, "Actual Position"=w1432:dbl)  [unwired: 7 in]
        n670 = Index Array(array=w1441, index=w1424) -> (element=w1443:T11)
        n671 = Unbundle By Name(w1443) -> ("Invert Direction X"=w1442:bool)
        n672 = call <vilib>:"Build State String with Arguments__jki_lib_state_machine.vi"("Arguments (\"\")"=w1437, "State"="Wait" ("State(s) in Front (\"\")")) -> ()  [unwired: 4 in, 1 out]
        n673 = call <vilib>:"Add State(s) to Queue__jki_lib_state_machine.vi"("State(s) in Front (\"\")"="RestartAveraging" ("State(s) in Front (\"\")"), "State(s) in (\"\")"=w1446) -> ("States Out"=w1445:string)  [unwired: 13 in]
        n674 = case shown="\"Left\", Default" w1436 {
          tunnel: w1442 -> [w1450 w1460]
          tunnel: "StepSize" -> [w1449 w1459]
          tunnel: w1432 -> [w1448 w1458]
          tunnel: [w1447 w1457] -> w1430
          frame "Right" {
            n675 = case shown="False" w1450 {
              tunnel: w1448 -> [w1453 w1456]
              tunnel: w1449 -> [w1452 w1455]
              tunnel: [w1451 w1454] -> w1447
              frame False {
                n676 = Add(x=w1453, y=w1452) -> (x+y=w1451:dbl)
              }
              frame True {
                n677 = Subtract(x=w1456, y=w1455) -> (x-y=w1454:dbl)
              }
            }
          }
          frame "Left", Default {
            n678 = case shown="True" w1460 {
              tunnel: w1458 -> [w1463 w1466]
              tunnel: w1459 -> [w1462 w1465]
              tunnel: [w1461 w1464] -> w1457
              frame False {
                n679 = Subtract(x=w1463, y=w1462) -> (x-y=w1461:dbl)
              }
              frame True {
                n680 = Add(x=w1466, y=w1465) -> (x+y=w1464:dbl)
              }
            }
          }
        }
        n681 = call "Beampointing get set motor position.vi"("Active CCD"=w1424, "error in (no error)"=w1422, "Set position"=w1430, "get or set"=enum16{"get", "set"}."set", "dev variable alias Motors X"=w1431) -> ("Actual Position"=w1425:dbl)  [unwired: 5 in, 1 out]
        n682 = Unbundle By Name(w1427) -> ("Motor positions.Positions x"=w1429:dbl[])
        n683 = Replace Array Subset(array=w1429, new element=w1425, index=w1424) -> (w1428:dbl[])
        n684 = Bundle By Name(cluster=w1427, "Motor positions.Positions x"=w1428) -> (w1426:T35)
      }
      frame "ManMove Y" {
        # "Your code here.\n(You can make a copy of, or modify, this frame)"
        n685 = Equal?(x=w1481, y="Down") -> ()  [unwired: 1 out]
        n686 = Unbundle By Name(w1470) -> ("active cams"=w1483:string[], "move properties"=w1487:T11[], "active ccd"=w1471:i32)
        n687 = Unbundle By Name(w1470) -> ("dev var alias arrays.dev variable alias Motors Y"=w1479:string[][])
        n688 = Index Array(array=w1483, index=w1471) -> (element=w1482:string)
        n689 = call "Beampointing get set motor position.vi"("Active CCD"=w1471, "get or set"=enum16{"get", "set"}."get", "dev variable alias Motors X"=w1479) -> ("Actual Position"=w1475:dbl)  [unwired: 7 in, 1 out]
        n690 = Index Array(array=w1487, index=w1471) -> (element=w1488:T11)
        n691 = property on="StepSize" class="DigNum (strict)"() -> ("Value"=w1484:dbl)  [unwired: 2 in, 2 out]
        n692 = Unbundle By Name(w1488) -> ("Invert Direction Y"=w1485:bool)
        n693 = call <vilib>:"Build State String with Arguments__jki_lib_state_machine.vi"("Arguments (\"\")"=w1482, "State"="Wait" ("State(s) in Front (\"\")")) -> ()  [unwired: 4 in, 1 out]
        n694 = case shown="\"Up\", Default" w1481 {
          tunnel: w1485 -> [w1495 w1505]
          tunnel: w1484 -> [w1494 w1504]
          tunnel: [w1493 w1502] -> w1476
          tunnel: w1475 -> [w1492 w1503]
          frame "Down" {
            n695 = case shown="False" w1495 {
              tunnel: w1492 -> [w1498 w1501]
              tunnel: w1494 -> [w1497 w1500]
              tunnel: [w1496 w1499] -> w1493
              frame False {
                n696 = Add(x=w1498, y=w1497) -> (x+y=w1496:dbl)
              }
              frame True {
                n697 = Subtract(x=w1501, y=w1500) -> (x-y=w1499:dbl)
              }
            }
          }
          frame "Up", Default {
            n698 = case shown="False" w1505 {
              tunnel: w1503 -> [w1508 w1511]
              tunnel: w1504 -> [w1507 w1510]
              tunnel: [w1506 w1509] -> w1502
              frame False {
                n699 = Subtract(x=w1508, y=w1507) -> (x-y=w1506:dbl)
              }
              frame True {
                n700 = Add(x=w1511, y=w1510) -> (x+y=w1509:dbl)
              }
            }
          }
        }
        n701 = call <vilib>:"Add State(s) to Queue__jki_lib_state_machine.vi"("State(s) in Front (\"\")"="RestartAveraging" ("State(s) in Front (\"\")"), "State(s) in (\"\")"=w1491) -> ("States Out"=w1490:string)  [unwired: 13 in]
        n702 = call "Beampointing get set motor position.vi"("Active CCD"=w1471, "Set position"=w1476, "get or set"=enum16{"get", "set"}."set", "dev variable alias Motors X"=w1479) -> ("Actual Position"=w1472:dbl)  [unwired: 6 in, 1 out]
        n703 = Unbundle By Name(w1470) -> ("Motor positions.Positions y"=w1474:dbl[])
        n704 = Replace Array Subset(array=w1474, new element=w1472, index=w1471) -> (w1473:dbl[])
        n705 = Bundle By Name(cluster=w1470, "Motor positions.Positions y"=w1473) -> (w1469:T35)
      }
      frame "Move Y" {
        # "Your code here.\n(You can make a copy of, or modify, this frame)"
        n706 = Unbundle By Name(w1523) -> ("dev var alias arrays.dev variable alias Motors Y"=w1524:string[][])
        n707 = Unbundle By Name(w1523) -> ("Offset Y"=w1536:dbl[][])
        n708 = call-poly <userlib>:"Filter 1D Array__ogtk.vi"("items to filter"=w1528, "array"=w1537) -> ("filtered item indices"=w1532:i32[])  [unwired: 4 in, 1 out]
        n709 = Unbundle By Name(w1523) -> ("move properties"=w1530:T11[])
        n710 = for {
          tunnel: w1532 -> [w1563] mode=indexing
          tunnel: w1530 -> [w1567]
          shift-right: [w1562] -> w1531
          shift-left: i32[] [] ("filtered item indices") -> [w1565]
          n711 = Index Array(array=w1567, index=w1563) -> (element=w1566:T11)
          n712 = Unbundle By Name(w1566) -> ("enable feedback"=w1564:bool)
          n713 = case shown="True" w1564 {
            tunnel: w1565 -> [w1568 w1571]
            tunnel: w1563 -> [_ w1570]
            tunnel: [w1568 w1569] -> w1562
            frame False {
            }
            frame True {
              n714 = Build Array (concatenate)(w1571, w1570) -> (w1569:i32[])
            }
          }
        }
        n715 = Index Array(array=w1531) -> (element=w1521:i32)  [unwired: 1 in]
        n716 = Index Array(array=w1536, index (row)=w1521) -> (element=w1535:dbl[])  [unwired: 1 in]
        n717 = Reverse 1D Array(array=w1535) -> (reversed array=w1534:dbl[])
        n718 = call "Beampointing get set motor position.vi"("Active CCD"=w1521, "error in (no error)"=w1517, "get or set"=enum16{"get", "set"}."get", "dev variable alias Motors X"=w1524) -> ("error out"=w1519:errorcluster, "Actual Position"=w1525:dbl)  [unwired: 6 in]
        n719 = Index Array(array=w1534) -> (element=w1516:dbl)  [unwired: 1 in]
        n720 = Index Array(array=w1530, index=w1521) -> (element=w1513:T11)
        n721 = Unbundle By Name(w1513) -> ("enable feedback"=w1533:bool)
        n722 = local read "Align"() -> (w1512:bool)
        n723 = call "relative move from offset and calibration.vi"("Align"=w1512, "axis"=enum16{"x", "y"}."y", "Offset"=w1516, "element"=w1513) -> ("relative move out"=w1515:dbl)  [unwired: 7 in]
        n724 = case shown="No Error" w1519 {
          selector: w1519 -> [_ w1560]
          tunnel: w1533 -> [w1550 _]
          tunnel: w1525 -> [w1549 _]
          tunnel: w1524 -> [w1548 _]
          tunnel: w1523 -> [w1545 w1561]
          tunnel: [w1544 w1561] -> w1522
          tunnel: w1521 -> [w1542 _]
          tunnel: w1515 -> [w1541 _]
          tunnel: [w1540 w1560] -> w1518
          frame No Error {
            n725 = case shown="True" w1550 {
              tunnel: w1541 -> [_ w1559]
              tunnel: w1549 -> [w1551 w1558]
              tunnel: w1548 -> [_ w1555]
              tunnel: w1542 -> [_ w1554]
              tunnel: [w1551 w1553] -> w1543
              tunnel: [_ w1552] -> w1540
              frame False {
              }
              frame True {
                n726 = Add(x=w1558, y=w1559) -> (x+y=w1557:dbl)
                n727 = call "Beampointing get set motor position.vi"("Active CCD"=w1554, "Set position"=w1557, "get or set"=enum16{"get", "set"}."set", "dev variable alias Motors X"=w1555) -> ("error out"=w1552:errorcluster, "Actual Position"=w1553:dbl)  [unwired: 6 in]
              }
            }
            n728 = Unbundle By Name(w1545) -> ("Motor positions.Positions y"=w1547:dbl[])
            n729 = Replace Array Subset(array=w1547, new element=w1543, index=w1542) -> (w1546:dbl[])
            n730 = Bundle By Name(cluster=w1545, "Motor positions.Positions y"=w1546) -> (w1544:T35)
          }
          frame Error {
          }
        }
        n731 = call <vilib>:"Build State String with Arguments__jki_lib_state_machine.vi"("Arguments (\"\")"=w1528, "State"="Wait" ("State(s) in Front (\"\")")) -> ()  [unwired: 4 in, 1 out]
        n732 = call <vilib>:"Add State(s) to Queue__jki_lib_state_machine.vi"("State(s) in (\"\")"=w1539) -> ("States Out"=w1538:string)  [unwired: 14 in]
        "Moving Y" <- w1528
      }
      frame "Wait" {
        # "Your code here.\n(You can make a copy of, or modify, this frame)"
        n733 = disable-structure shown="Disabled" {
          disable-tunnel: w1577 -> [w1591 _]
          disable-tunnel: w1576 -> [w1590 _]
          disable-tunnel: w1575 -> [w1589 _]
          disable-tunnel: w1574 -> [w1587 w1611]
          disable-tunnel: [w1586 w1611] -> w1573
          frame Disabled {
            n734 = call-poly <userlib>:"Filter 1D Array__ogtk.vi"("items to filter"=w1589, "array"=w1590) -> ("filtered item indices"=w1588:i32[])  [unwired: 4 in, 1 out]
            n735 = Index Array(array=w1588) -> (element=w1585:i32)  [unwired: 1 in]
            n736 = flat-sequence {
              tunnel: T30."Disabled and Grayed Out" ("Disabled") -> [w1592]
              tunnel: w1587 -> [w1600]
              tunnel: [w1599] -> w1586
              tunnel: w1585 -> [w1598]
              tunnel: w1584 -> [w1597]
              tunnel: T30."Enabled" ("Disabled") -> [w1610]
              frame #0 {
                n737 = property on="Right" class="Bool (strict)"("DisabledEnum"=w1592) -> ()  [unwired: 2 in, 2 out]
                n738 = property on="Up" class="Bool (strict)"("DisabledEnum"=w1592) -> ()  [unwired: 2 in, 2 out]
                n739 = property on="Left" class="Bool (strict)"("DisabledEnum"=w1592) -> ()  [unwired: 2 in, 2 out]
                n740 = property on="Down" class="Bool (strict)"("DisabledEnum"=w1592) -> ()  [unwired: 2 in, 2 out]
                n741 = property on="StepSize" class="DigNum (strict)"("DisabledEnum"=w1592) -> ()  [unwired: 2 in, 2 out]
              }
              frame #1 {
                n742 = Wait (ms)(milliseconds to wait=u32 1500) -> ()  [unwired: 1 out]
              }
              frame #2 {
                n743 = property on="Moving Y" class="Str"("Value"="") -> ()  [unwired: 2 in, 2 out]
                n744 = property on="Moving X" class="Str"("Value"="") -> ()  [unwired: 2 in, 2 out]
              }
              frame #3 {
                n745 = Equal?(x=w1597, y=w1598) -> (x = y?=w1596:bool)
                n746 = case shown="True" w1596 {
                  tunnel: _ -> [_ w1607]
                  tunnel: w1600 -> [w1601 w1604]
                  tunnel: [w1601 w1602] -> w1599
                  frame False {
                  }
                  frame True {
                    n747 = Unbundle By Name(w1607) -> ("Ref X"=w1606, "Ref Y"=w1605)
                    n748 = property class="DigNum (strict)"(reference=w1606, error in=w1604) -> (error out=w1603:errorcluster, "Value"=w1609:dbl)  [unwired: 1 out]
                    n749 = property class="DigNum (strict)"(reference=w1605, error in=w1603) -> (error out=w1602:errorcluster, "Value"=w1608:dbl)  [unwired: 1 out]
                    n750 = property on="Position 1" class="DigNum (strict)"("Value"=w1609) -> ()  [unwired: 2 in, 2 out]
                    n751 = property on="Position 2" class="DigNum (strict)"("Value"=w1608) -> ()  [unwired: 2 in, 2 out]
                  }
                }
              }
              frame #4 {
                n752 = property on="Right" class="Bool (strict)"("DisabledEnum"=w1610) -> ()  [unwired: 2 in, 2 out]
                n753 = property on="Up" class="Bool (strict)"("DisabledEnum"=w1610) -> ()  [unwired: 2 in, 2 out]
                n754 = property on="Left" class="Bool (strict)"("DisabledEnum"=w1610) -> ()  [unwired: 2 in, 2 out]
                n755 = property on="Down" class="Bool (strict)"("DisabledEnum"=w1610) -> ()  [unwired: 2 in, 2 out]
                n756 = property on="StepSize" class="DigNum (strict)"("DisabledEnum"=w1610) -> ()  [unwired: 2 in, 2 out]
              }
            }
            n757 = Unbundle By Name(w1591) -> ("active ccd"=w1584:i32)
          }
          frame Enabled {
          }
        }
        n758 = call <vilib>:"Add State(s) to Queue__jki_lib_state_machine.vi"("State(s) in (\"\")"=w1581) -> ("States Out"=w1580:string)  [unwired: 14 in]
        n759 = local read "Mean Centroid X"() -> (w1578:dbl[][])
        n760 = Bundle By Name(cluster=w1577, "Mean Centroid X"=w1578, "Mean Centroid Y"=w1578) -> (w1579:T35)
      }
      frame "RestartAveraging" {
        # "clear arrays"
        n761 = Unbundle By Name(w1618) -> ("Detection"=w1619:T32)
        n762 = Unbundle By Name(w1619) -> ("img to avg"=w1621:i32)
        n763 = Decrement(x=w1621) -> (x-1=w1616:i32)
        n764 = Initialize Array(0.0 ("element"), 12 ("dimension size"), w1616) -> (w1613:dbl[][])
        n765 = Bundle By Name(cluster=w1619, "Centroid X"=w1613, "Centroid Y"=w1613, "Size"=w1613) -> (w1620:T32)
        n766 = Bundle By Name(cluster=w1618, "Detection"=w1620) -> (w1617:T35)
        n767 = local write "#imgs avd so far"(0.0 ("#imgs avd so far")) -> ()
        n768 = call <vilib>:"Add State(s) to Queue__jki_lib_state_machine.vi"("State(s) in (\"\")"=w1625) -> ("States Out"=w1624:string)  [unwired: 14 in]
      }
      frame "---------------Statistics--------------" {
        # "Template Separator\n(You can make a copy of, or modify, this frame)"
        n769 = call <vilib>:"Add State(s) to Queue__jki_lib_state_machine.vi"("State(s) in (\"\")"=w1630) -> ("States Out"=w1629:string)  [unwired: 14 in]
      }
      frame "Save Stats" {
        # "Your code here.\n(You can make a copy of, or modify, this frame)"
        n770 = disable-structure shown="Disabled" {
          disable-tunnel: w1637 -> [w1641 _]
          disable-tunnel: [w1640 _] -> w1636
          disable-tunnel: _ -> [w1639 _]
          disable-tunnel: w1633 -> [w1638 _]
          frame Disabled {
            n771 = for {
              tunnel: w1639 -> [w1644] mode=indexing
              tunnel: w1638 -> [w1643] mode=indexing
              n772 = Empty String/Path?(string/path=w1643) -> (empty?=w1642:bool)
              n773 = case shown="False" w1642 {
                tunnel: w1644 -> [w1650 _]
                tunnel: w1643 -> [w1648 _]
                frame False {
                  n774 = Index Array(array=w1650, index #1=0 ("index"), index #2=1 ("index"), index #3=2 ("index"), index #4=3 ("index")) -> (element #1=w1685, element #2=w1679, element #3=w1678, element #4=w1677)  [unwired: 1 in, 1 out]
                  n775 = Concatenate Strings(w1648, ".dat" ("string")) -> (w1646:string)
                  n776 = Unbundle(w1685) -> (w1684, w1662)
                  n777 = Unbundle(w1679) -> (w1653)  [unwired: 1 out]
                  n778 = Unbundle(w1678) -> (w1652)  [unwired: 1 out]
                  n779 = Unbundle(w1677) -> (w1651)  [unwired: 1 out]
                  n780 = Build Path(base path="save path", name or relative path=w1646) -> (appended path=w1645:path)
                  n781 = for {
                    tunnel: w1684 -> [w1687]
                    tunnel: [w1686] -> w1660 mode=indexing
                    n782 = Format Date/Time String(time format string (%c)="%Y%m%d%H%M%S", seconds (now)=w1687) -> (date/time string=w1686:string)  [unwired: 1 in]
                  }
                  n783 = Array Size(array=w1662) -> (size(s)=w1663:i32)
                  n784 = Number To Fractional String(number=w1662) -> (F-format string=w1659:string)  [unwired: 3 in]
                  n785 = Number To Fractional String(number=w1653) -> (F-format string=w1656:string)  [unwired: 3 in]
                  n786 = Number To Fractional String(number=w1652) -> (F-format string=w1655:string)  [unwired: 3 in]
                  n787 = Number To Fractional String(number=w1651) -> (F-format string=w1654:string)  [unwired: 3 in]
                  n788 = Initialize Array("", w1663, 5 ("dimension size")) -> (w1661:string[][])
                  n789 = Insert Into Array(array=w1661, index (col)=0 ("disabled index (col)"), new element=w1660) -> (w1671:string[][])  [unwired: 1 in]
                  n790 = Insert Into Array(array=w1671, index (col)=1 ("disabled index (col)"), new element=w1659) -> (w1670:string[][])  [unwired: 1 in]
                  n791 = Insert Into Array(array=w1670, index (col)=2 ("disabled index (col)"), new element=w1656) -> (w1674:string[][])  [unwired: 1 in]
                  n792 = Insert Into Array(array=w1674, index (col)=3 ("disabled index (col)"), new element=w1655) -> (w1675:string[][])  [unwired: 1 in]
                  n793 = Insert Into Array(array=w1675, index (col)=4 ("disabled index (col)"), new element=w1654) -> (w1676:string[][])  [unwired: 1 in]
                  n794 = Insert Into Array(array=w1676, index (row)=0, new element=string[] ["time", "Centroid X", "Centroid Y", "Motor Axis 1", "Motor Axis 2"] ("new element/subarray 2")) -> (w1658:string[][])  [unwired: 1 in]
                  n795 = call-poly <vilib>:"Write To Spreadsheet File.vi"("2D data"=w1658, "file path (dialog if empty)"=w1645) -> ()  [unwired: 6 in, 1 out]
                }
                frame True {
                }
              }
            }
            n796 = call <vilib>:"Add State(s) to Queue__jki_lib_state_machine.vi"("State(s) in (\"\")"=w1641) -> ("States Out"=w1640:string)  [unwired: 14 in]
          }
          frame Enabled {
          }
        }
        n797 = property on="Save Stats" class="Bool (strict)"("Value"=FALSE ("Save Stats")) -> ()  [unwired: 2 in, 2 out]
      }
      frame "tdms" {
        w1702 = 21600.0 ("new tdms")
        # "Your code here.\n(You can make a copy of, or modify, this frame)"
        n798 = Unbundle By Name(w1709) -> ("active cams"=w1695:string[], "tdms ref"=w1692:refnum<k34>, "Offset X"=w1708:dbl[][], "Offset Y"=w1707:dbl[][], "Motor positions.Positions x"=w1690:dbl[], "Motor positions.Positions y"=w1689:dbl[])
        n799 = for {
          tunnel: w1708 -> [w1752]
          tunnel: w1707 -> [w1751]
          tunnel: w1695 -> [w1724] mode=indexing
          tunnel: w1692 -> [w1725]
          tunnel: w1711 -> [w1719]
          tunnel: [w1728] -> w1710
          tunnel: w1690 -> [w1718]
          tunnel: w1689 -> [w1716]
          i -> [w1715]
          n800 = Index Array(array=w1752, index (row)=w1715) -> (element=w1750:dbl[])  [unwired: 1 in]
          n801 = Index Array(array=w1751, index (row)=w1715) -> (element=w1749:dbl[])  [unwired: 1 in]
          n802 = Reverse 1D Array(array=w1749) -> (reversed array=w1747:dbl[])
          n803 = Reverse 1D Array(array=w1750) -> (reversed array=w1748:dbl[])
          n804 = Index Array(array=w1748) -> (element=w1746:dbl)  [unwired: 1 in]
          n805 = Index Array(array=w1747) -> (element=w1745:dbl)  [unwired: 1 in]
          n806 = Index Array(array=w1716, index=w1715) -> (element=w1714:dbl)
          n807 = Index Array(array=w1718, index=w1715) -> (element=w1717:dbl)
          n808 = Build Array(w1746) -> (w1727:dbl[])
          n809 = Build Array(w1745) -> (w1740:dbl[])
          n810 = Get Date/Time In Seconds() -> (seconds since 1Jan1904=w1726:timestamp)
          n811 = Build Array(w1726) -> (w1722:timestamp[])
          n812 = Build Array(w1717) -> (w1734:dbl[])
          n813 = TDMS Write(0:w1725, 5:w1724, 7:"time", 9:w1722, 11:w1719) -> (4:w1721:refnum<k34>, 15:w1720:errorcluster)  [unwired: 1 in, 2 out]
          n814 = Build Array(w1714) -> (w1729:dbl[])
          n815 = TDMS Write(0:w1721, 5:w1724, 7:"centroid X", 9:w1727, 11:w1720) -> (4:w1743:refnum<k34>, 6:w1742:string, 15:w1741:errorcluster)  [unwired: 1 in, 1 out]
          n816 = TDMS Write(0:w1743, 5:w1742, 7:"centroid Y", 9:w1740, 11:w1741) -> (4:w1737:refnum<k34>, 6:w1736:string, 15:w1738:errorcluster)  [unwired: 1 in, 1 out]
          n817 = TDMS Write(0:w1737, 5:w1736, 7:"Motor Axis 1", 9:w1734, 11:w1738) -> (4:w1733:refnum<k34>, 6:w1732:string, 15:w1730:errorcluster)  [unwired: 1 in, 1 out]
          n818 = TDMS Write(0:w1733, 5:w1732, 7:"Motor Axis 2", 9:w1729, 11:w1730) -> (15:w1728:errorcluster)  [unwired: 1 in, 3 out]
        }
        n819 = property on="millisecond timer value" class="DigNum (strict)"() -> ("Value"=w1694:u32)  [unwired: 2 in, 2 out]
        n820 = Tick Count (ms)() -> (millisecond timer value=w1693:u32)
        n821 = Unbundle By Name(w1709) -> ()  [unwired: 1 out]
        n822 = Subtract(x=w1693, y=w1694) -> (x-y=w1697:u32)
        n823 = Divide(x=w1697, y=u32 1000) -> (x/y=w1699:dbl)
        n824 = Quotient & Remainder(x=w1699, y=w1702) -> (x-y*floor(x/y)=w1700:dbl)  [unwired: 1 out]
        n825 = Subtract(x=w1702, y=20.0) -> (x-y=w1704:dbl)
        n826 = Greater?(x=w1700, y=w1704) -> (0:w1701:bool)
        n827 = Select(t="newtdms", s=w1701, f="") -> (s? t:f=w1696:string)
        n828 = call <vilib>:"Add State(s) to Queue__jki_lib_state_machine.vi"("State(s) in (\"\")"=w1713, "State(s) at Back (\"\")"=w1696) -> ("States Out"=w1712:string)  [unwired: 13 in]
      }
      frame "Reset History" {
        # "Your code here.\n(You can make a copy of, or modify, this frame)"
        n829 = for {
          N: 1 -> [_]
          shift-right: [w1763] -> w1755
          shift-left: timestamp[][] [] ("Time") -> [w1765]
          n830 = for {
            N: 12 -> [_]
            tunnel: w1765 -> [w1768] mode=indexing
            tunnel: [w1766] -> w1763 mode=indexing
            n831 = Get Date/Time In Seconds() -> (seconds since 1Jan1904=w1767:timestamp)
            n832 = Build Array (concatenate)(w1768, w1767) -> (w1766:timestamp[])
          }
        }
        n833 = local read "Offset X"() -> (w1754:dbl[][])
        n834 = Bundle By Name(cluster=w1759, "Offset X"=w1754, "Offset Y"=w1754, "Time"=w1755, "Motor X"=w1754) -> (w1758:T35)
        n835 = call <vilib>:"Add State(s) to Queue__jki_lib_state_machine.vi"("State(s) in (\"\")"=w1762) -> ("States Out"=w1761:string)  [unwired: 14 in]
      }
      frame "New Category: 2" {
        # "Your code here.\n(You can make a copy of, or modify, this frame)"
        n836 = call <vilib>:"Add State(s) to Queue__jki_lib_state_machine.vi"("State(s) in (\"\")"=w1773) -> ("States Out"=w1772:string)  [unwired: 14 in]
      }
      frame "stats" {
        # "Your code here.\n(You can make a copy of, or modify, this frame)"
        n837 = Unbundle By Name(w1789) -> ("Offset X"=w1780:dbl[][], "Offset Y"=w1779:dbl[][], "Time"=w1778:timestamp[][], "Motor X"=w1777:dbl[][], "Motor Y"=w1776:dbl[][], "tdms ref"=w1784:refnum<k34>)
        n838 = TDMS List Contents(4:w1783, 7:w1784) -> (0:w1775:errorcluster, 2:w1787:string[], 3:w1786:refnum<k34>)  [unwired: 1 in, 1 out]
        n839 = call <vilib>:"ClearError.vi"("error in (no error)"=w1775) -> ("error out"=w1785:errorcluster)
        n840 = for {
          tunnel: w1785 -> [w1834]
          tunnel: [w1820] -> w1781 mode=indexing
          tunnel: [w1819] -> w1782
          tunnel: [w1818] -> _
          tunnel: w1786 -> [w1817]
          tunnel: w1787 -> [w1816] mode=indexing
          w1835 = dbl[] [] ("appended array")
          n841 = TDMS Read(0:w1817, 5:w1816, 7:"time", 11:w1834, 12:timestamp[] [] ("appended array")) -> (4:w1849:refnum<k34>, 6:w1845:string, 10:w1826:timestamp[], 15:w1833:errorcluster)  [unwired: 3 in, 2 out]
          n842 = TDMS Read(0:w1849, 5:w1845, 7:"centroid X", 11:w1833, 12:w1835) -> (4:w1848:refnum<k34>, 6:w1844:string, 10:w1829:dbl[], 15:w1832:errorcluster)  [unwired: 3 in, 2 out]
          n843 = TDMS Read(0:w1848, 5:w1844, 7:"centroid Y", 11:w1832, 12:w1835) -> (4:w1847:refnum<k34>, 6:w1843:string, 10:w1828:dbl[], 15:w1831:errorcluster)  [unwired: 3 in, 2 out]
          n844 = TDMS Read(0:w1847, 5:w1843, 7:"Motor Axis 1", 11:w1831, 12:w1835) -> (4:w1846:refnum<k34>, 6:w1842:string, 10:w1827:dbl[], 15:w1830:errorcluster)  [unwired: 3 in, 2 out]
          n845 = TDMS Read(0:w1846, 5:w1842, 7:"Motor Axis 2", 11:w1830, 12:w1835) -> (4:w1818:refnum<k34>, 10:w1825:dbl[], 15:w1819:errorcluster)  [unwired: 3 in, 3 out]
          n846 = Bundle("appended array"=w1826, "appended array"=w1829) -> (w1824:T56)  [unwired: 1 in]
          n847 = Bundle("appended array"=w1826, "appended array"=w1828) -> (w1823:T56)  [unwired: 1 in]
          n848 = Bundle("appended array"=w1826, "appended array"=w1827) -> (w1822:T56)  [unwired: 1 in]
          n849 = Bundle("appended array"=w1826, "appended array"=w1825) -> (w1821:T56)  [unwired: 1 in]
          n850 = Build Array(w1824, w1823, w1822, w1821) -> (w1820:T57)
        }
        n851 = disable-structure shown="Disabled" {
          disable-tunnel: w1788 -> [w1799 _]
          disable-tunnel: w1780 -> [w1798 _]
          disable-tunnel: w1779 -> [w1797 _]
          disable-tunnel: w1778 -> [w1796 _]
          disable-tunnel: w1777 -> [w1795 _]
          disable-tunnel: w1776 -> [w1794 _]
          frame Disabled {
            n852 = for {
              tunnel: w1799 -> [_] mode=indexing
              tunnel: w1798 -> [w1809]
              tunnel: w1797 -> [w1808]
              tunnel: w1796 -> [w1807]
              tunnel: w1795 -> [w1803]
              tunnel: w1794 -> [w1802]
              tunnel: [w1811] -> _ mode=indexing
              i -> [w1810]
              n853 = Index Array(array=w1808, index (row)=w1810) -> (element=w1804:dbl[])  [unwired: 1 in]
              n854 = Index Array(array=w1803, index (row)=w1810) -> (element=w1801:dbl[])  [unwired: 1 in]
              n855 = Index Array(array=w1802, index (row)=w1810) -> (element=w1800:dbl[])  [unwired: 1 in]
              n856 = Index Array(array=w1809, index (row)=w1810) -> (element=w1805:dbl[])  [unwired: 1 in]
              n857 = Index Array(array=w1807, index (row)=w1810) -> (element=w1806:timestamp[])  [unwired: 1 in]
              n858 = Bundle("Time"=w1806, "Motor X"=w1801) -> (w1814:cluster{"Time":timestamp[], "Motor X":dbl[]})  [unwired: 1 in]
              n859 = Bundle("Time"=w1806, "Motor Y"=w1800) -> (w1815:cluster{"Time":timestamp[], "Motor Y":dbl[]})  [unwired: 1 in]
              n860 = Bundle("Time"=w1806, "Offset X"=w1805) -> (w1813:cluster{"Time":timestamp[], "Offset X":dbl[]})  [unwired: 1 in]
              n861 = Bundle("Time"=w1806, "Offset Y"=w1804) -> (w1812:cluster{"Time":timestamp[], "Offset Y":dbl[]})  [unwired: 1 in]
              n862 = Build Array(w1812, w1813, w1814, w1815) -> (w1811:cluster{"Time":timestamp[], "Motor Y":dbl[]}[])
            }
          }
          frame Enabled {
          }
        }
        n863 = Index Array(array=w1781, index (row)="Cam# history") -> (element=→"CCD 1":T57)  [unwired: 1 in]
        n864 = call <vilib>:"Add State(s) to Queue__jki_lib_state_machine.vi"("State(s) in (\"\")"=w1793) -> ("States Out"=w1792:string)  [unwired: 14 in]
      }
      frame "newtdms" {
        n865 = Unbundle By Name(w1888) -> ("tdms ref"=w1881:refnum<k34>, "active cams"=w1876:string[])
        n866 = Empty String/Path?(string/path="tdms root") -> (empty?=w1853:bool)
        n867 = Select(t=path "c:/BeamPointing" ("tdms root"), s=w1853, f="tdms root") -> (s? t:f=w1850:path)
        n868 = TDMS Close(8:w1886, 11:w1881) -> (0:w1875:errorcluster)  [unwired: 1 out]
        n869 = local read "config path"() -> (w1857:string)
        n870 = call <vilib>:"Clear Errors.vi"("error in (no error)"=w1875) -> ("error out"=w1864:errorcluster)  [unwired: 5 in, 1 out]
        n871 = Get Date/Time In Seconds() -> (seconds since 1Jan1904=w1869:timestamp)
        n872 = call-poly <userlib>:"Strip Path Extension__ogtk.vi"("path"=w1857) -> ("root"=w1856:string)  [unwired: 1 out]
        n873 = property on="new tdms" class="Bool (strict)"("Value"=FALSE ("new tdms")) -> ()  [unwired: 2 in, 2 out]
        n874 = Format Date/Time String(time format string (%c)="%Y%m%d", seconds (now)=w1869) -> (date/time string=w1870:string)  [unwired: 1 in]
        n875 = Format Date/Time String(time format string (%c)="%Y%m%d%H%M", seconds (now)=w1869) -> (date/time string=w1867:string)  [unwired: 1 in]
        n876 = String To Path(string=w1856) -> (path=w1855:path)
        n877 = Strip Path(path=w1855) -> (name=w1854:string)  [unwired: 1 out]
        n878 = Build Path(base path=w1850, name or relative path=w1870) -> (appended path=w1871:path)
        n879 = Concatenate Strings(w1867, w1854, ".tdms" ("string")) -> (w1866:string)
        n880 = String To Path(string=w1866) -> (path=w1862:path)
        n881 = call <vilib>:"Check if File or Folder Exists.vi"("error in (no error)"=w1864, "path"=w1871) -> ("error out"=w1874:errorcluster, "file or folder exists?"=w1872:bool, "dup path"=w1873:path)  [unwired: 7 in]
        n882 = case shown="False" w1872 {
          tunnel: w1873 -> [w1894 w1896]
          tunnel: [w1893 w1896] -> w1861
          tunnel: w1874 -> [w1892 w1895]
          tunnel: [w1891 w1895] -> w1863
          frame False {
            n883 = Create Folder(path (use dialog)=w1894, error in=w1892) -> (created path=w1893:path, error out=w1891:errorcluster)  [unwired: 1 in, 1 out]
          }
          frame True {
          }
        }
        n884 = call <vilib>:"Add State(s) to Queue__jki_lib_state_machine.vi"("State(s) in (\"\")"=w1890) -> ("States Out"=w1889:string)  [unwired: 14 in]
        n885 = Build Path(base path=w1861, name or relative path=w1862) -> (appended path=w1882:path)
        n886 = TDMS Open(6:FALSE ("disable buffering (T)"), 7:enum16{"1.0", "2.0"}."2.0" ("file format version (2.0)"), 8:w1863, 10:T31."create or replace" ("operation"), 11:w1882) -> (0:w1879:errorcluster, 3:w1878:refnum<k34>)  [unwired: 2 in]
        n887 = call "TDMSbuffersize.vi"("error in (no error)"=w1879, "group names"=w1876, "Data Value Reference in"=w1878) -> ("error out"=w1859:errorcluster, "Data Value Reference out"=w1877:refnum<k34>)  [unwired: 7 in]
        n888 = Bundle By Name(cluster=w1888, "tdms ref"=w1877) -> (w1887:T35)
      }
      frame "Center" {
        # "Your code here.\n(You can make a copy of, or modify, this frame)"
        n889 = control-ref of="image::1"() -> (w1912:refnum<vi>)
        n890 = control-ref of="image::2"() -> (w1911:refnum<vi>)
        n891 = control-ref of="image::3"() -> (w1910:refnum<vi>)
        n892 = control-ref of="image::4"() -> (w1909:refnum<vi>)
        n893 = control-ref of="image::5"() -> (w1908:refnum<vi>)
        n894 = control-ref of="image::6"() -> (w1907:refnum<vi>)
        n895 = control-ref of="image::7"() -> (w1906:refnum<vi>)
        n896 = control-ref of="image::8"() -> (w1905:refnum<vi>)
        n897 = control-ref of="image::9"() -> (w1904:refnum<vi>)
        n898 = control-ref of="image::10"() -> (w1903:refnum<vi>)
        n899 = control-ref of="image::11"() -> (w1902:refnum<vi>)
        n900 = control-ref of="image::12"() -> (w1901:refnum<vi>)
        n901 = for {
          tunnel: [w1921] -> w1900 mode=indexing
          tunnel: w1899 -> [w1920] mode=indexing
          n902 = Unbundle By Name(w1920) -> ("Target.X::12"=w1919:refnum<vi>, "Target.Y::12"=w1918:refnum<vi>)
          n903 = property class="DigNum (strict)"(reference=w1919) -> ("Value"=w1922:dbl)  [unwired: 1 in, 2 out]
          n904 = property class="DigNum (strict)"(reference=w1918) -> ("Value"=w1923:dbl)  [unwired: 1 in, 2 out]
          n905 = Bundle("Value"=w1922, "Value"=w1923) -> (w1921:cluster{"Value":dbl, "Value":dbl})  [unwired: 1 in]
        }
        n906 = call <vilib>:"Add State(s) to Queue__jki_lib_state_machine.vi"("State(s) in (\"\")"=w1917) -> ("States Out"=w1916:string)  [unwired: 14 in]
        n907 = Build Array(w1912, w1911, w1910, w1909, w1908, w1907, w1906, w1905, w1904, w1903, w1902, w1901) -> (w1913:refnum<vi>[])
        n908 = for {
          tunnel: w1913 -> [w1925] mode=indexing
          tunnel: w1900 -> [w1924] mode=indexing
          n909 = property class="ImageControl"(reference=w1925, "Image Center Position"=w1924) -> ()  [unwired: 1 in, 2 out]
        }
        n910 = property on="Center" class="Bool (strict)"("Value"=FALSE ("Center")) -> ()  [unwired: 2 in, 2 out]
      }
      frame "ImgToAvg" {
        n911 = Bundle By Name(cluster=w1935, "Detection.img to avg"="img to avg") -> (w1934:T35)
        n912 = call <vilib>:"Build State String with Arguments__jki_lib_state_machine.vi"("Arguments (\"\")"="T" ("Arguments (\"\")"), "State"=" Device Ini") -> ("State with Arguments"=w1928:string)  [unwired: 4 in]
        n913 = call <vilib>:"Add State(s) to Queue__jki_lib_state_machine.vi"("State(s) in Front (\"\")"=w1928, "State(s) in (\"\")"=w1933) -> ("States Out"=w1932:string)  [unwired: 13 in]
      }
      frame "history" {
        # "Your code here.\n(You can make a copy of, or modify, this frame)"
        n914 = Unbundle By Name(w1946) -> ("Offset X"=w1952:dbl[][], "Offset Y"=w1951:dbl[][], "Mean Centroid X"=w1950:dbl[][], "Mean Centroid Y"=w1949:dbl[][], "Motor X"=w1948:dbl[][], "Motor Y"=w1947:dbl[][], "Time"=w1938:timestamp[][])
        n915 = for {
          tunnel: w1952 -> [w1970] mode=indexing
          tunnel: w1951 -> [w1968] mode=indexing
          tunnel: w1950 -> [w1967] mode=indexing
          tunnel: w1949 -> [w1966] mode=indexing
          tunnel: w1948 -> [w1965] mode=indexing
          tunnel: w1947 -> [w1964] mode=indexing
          tunnel: [w1969] -> w1944 mode=indexing
          tunnel: [w1963] -> w1943 mode=indexing
          tunnel: [w1959] -> w1942 mode=indexing
          tunnel: [w1962] -> w1941 mode=indexing
          tunnel: [w1961] -> w1940 mode=indexing
          tunnel: [w1960] -> w1939 mode=indexing
          tunnel: w1938 -> [w1958] mode=indexing
          tunnel: [w1956] -> w1937 mode=indexing
          w1957 = 0
          n916 = Delete From Array(array=w1965, index=w1957) -> (array with subset deleted=w1961:dbl[])  [unwired: 1 in, 1 out]
          n917 = Delete From Array(array=w1964, index=w1957) -> (array with subset deleted=w1960:dbl[])  [unwired: 1 in, 1 out]
          n918 = Delete From Array(array=w1958, index=w1957) -> (array with subset deleted=w1956:timestamp[])  [unwired: 1 in, 1 out]
          n919 = Delete From Array(array=w1967, index=w1957) -> (array with subset deleted=w1959:dbl[])  [unwired: 1 in, 1 out]
          n920 = Delete From Array(array=w1966, index=w1957) -> (array with subset deleted=w1962:dbl[])  [unwired: 1 in, 1 out]
          n921 = Delete From Array(array=w1968, index=w1957) -> (array with subset deleted=w1963:dbl[])  [unwired: 1 in, 1 out]
          n922 = Delete From Array(array=w1970, index=w1957) -> (array with subset deleted=w1969:dbl[])  [unwired: 1 in, 1 out]
        }
        n923 = call <vilib>:"Add State(s) to Queue__jki_lib_state_machine.vi"("State(s) in (\"\")"=w1955) -> ("States Out"=w1954:string)  [unwired: 14 in]
        n924 = Bundle By Name(cluster=w1946, "Offset X"=w1944, "Offset Y"=w1943, "Mean Centroid X"=w1942, "Mean Centroid Y"=w1941, "Motor X"=w1940, "Motor Y"=w1939, "Time"=w1937) -> (w1945:T35)
      }
    }
    "Prev State" <- w49
    n925 = property on="Box" class="Arr (strict)"() -> ("Value"=w57:T2)  [unwired: 2 in, 2 out]
    n926 = for {
      tunnel: w58 -> [w101]
      tunnel: w51 -> [w110]
      tunnel: w55 -> [w108] mode=indexing
      tunnel: w57 -> [w69] mode=indexing
      tunnel: w54 -> [w99]
      tunnel: w53 -> [w98]
      tunnel: w52 -> [w80]
      i -> [w79]
      w94 = T58 {"Draw"=TRUE, "Target"={"x"=20.0, "y"=20.0}, "Size"={"x"=20.0, "y"=20.0}, "Angle"=1250067.0, "Color"=1250067, "Thickness"=0, "CrosshairLabel"=""} ("Crosshair")
      w88 = T59 {"Left"=0, "Top"=0, "Right"=0, "Bottom"=0} ("Bounding Rectangle")
      n927 = call-poly <userlib>:"Filter 1D Array__ogtk.vi"("items to filter"=w108, "array"=w110) -> ("filtered item indices"=w111:i32[])  [unwired: 4 in, 1 out]
      n928 = Index Array(array=w111) -> (element=w100:i32)  [unwired: 1 in]
      n929 = Index Array(array=w80, index (row)=w79) -> (element=w77:dbl[])  [unwired: 1 in]
      n930 = Index Array(array=w99, index (row)=w79) -> (element=w87:dbl[])  [unwired: 1 in]
      n931 = Index Array(array=w98, index (row)=w79) -> (element=w85:dbl[])  [unwired: 1 in]
      n932 = Index Array(array=w101, index=w100) -> (element=w109:T20)
      n933 = Reverse 1D Array(array=w77) -> (reversed array=w76:dbl[])
      n934 = Unbundle By Name(w109) -> ("Target.X::12"=w113:refnum<vi>, "Target.Y::12"=w112:refnum<vi>)
      n935 = Reverse 1D Array(array=w87) -> (reversed array=w86:dbl[])
      n936 = Reverse 1D Array(array=w85) -> (reversed array=w84:dbl[])
      n937 = Index Array(array=w76) -> (element=w74:dbl)  [unwired: 1 in]
      n938 = Square Root(x=w74) -> (sqrt(x)=w73:dbl)
      n939 = Index Array(array=w84) -> (element=w81:dbl)  [unwired: 1 in]
      n940 = Index Array(array=w86) -> (element=w82:dbl)  [unwired: 1 in]
      n941 = Divide(x=w73, y=2.0) -> (x/y=w71:dbl)
      n942 = property class="DigNum (strict)"(reference=w113) -> ("Value"=w105:dbl)  [unwired: 1 in, 2 out]
      n943 = property class="DigNum (strict)"(reference=w112) -> ("Value"=w104:dbl)  [unwired: 1 in, 2 out]
      n944 = Bundle(cluster=cluster{"xhair size":dbl, "xhair size 2":dbl} {"xhair size"=25.0, "xhair size 2"=25.0} ("size"), "xhair size"=w71, "xhair size 2"=w71) -> (w75:cluster{"xhair size":dbl, "xhair size 2":dbl})
      n945 = Bundle By Name(cluster=w94, "Draw"=TRUE, "Target.x"=w105, "Target.y"=w104, "Size"=w75, "Color"=u32 16774656, "Angle"=0.0, "Thickness"=u8 1) -> (w107:T58)
      n946 = call "draw crosshair imaq.vi"("clear overlay"=TRUE, "Crosshair"=w107, "Bounding Rectangle"=w88, "image in"=w108) -> ("error out"=w91:errorcluster, "image out"=w90:T5)  [unwired: 6 in]
      n947 = Bundle By Name(cluster=w94, "Draw"=TRUE, "Target.x"=w82, "Target.y"=w81, "Size"=w75, "Color"=u32 8322834, "Angle"=0.0, "Thickness"=u8 1) -> (w92:T58)
      n948 = case shown="True" "average centroid" {
        tunnel: w92 -> [_ w118]
        tunnel: w91 -> [_ w123]
        tunnel: w90 -> [w115 w122]
        tunnel: w88 -> [_ w121]
        tunnel: w69 -> [w116 _]
        tunnel: [w114 w120] -> w68
        frame False {
          n949 = call "draw box imaq.vi"("Color"=u32 1244928, "Rectangle"=w116, "image in"=w115) -> ("error out"=w114:errorcluster)  [unwired: 7 in, 1 out]
        }
        frame True {
          n950 = call "draw crosshair imaq.vi"("clear overlay"=FALSE, "error in (no error)"=w123, "Crosshair"=w118, "Bounding Rectangle"=w121, "image in"=w122) -> ("error out"=w120:errorcluster)  [unwired: 5 in, 1 out]
        }
      }
      "error out 3" <- w68
    }
  }
  n951 = call <userlib>:"Fit VI window to Largest Dec__ogtk.vi"() -> ()  [unwired: 6 in, 2 out]
  n952 = disable-structure shown="Enabled" {
    frame Disabled {
      # "GetMotorPositions"
      # "get all motor positions"
      n953 = call <userlib>:"Tick Count (ms)__ogtk.vi"() -> ("millisecond timer value"=w1979:u32)  [unwired: 10 in, 1 out]
      n954 = Unbundle By Name(w1980) -> ("dev var alias arrays"=w1972)
      n955 = Unbundle By Name(w1972) -> ("dev variable alias Motors X"=w1971, "dev variable alias Motors Y"=w1975)
      n956 = for {
        tunnel: w1975 -> [w1988]
        tunnel: w1971 -> [w1987]
        tunnel: [w1983] -> w1973 mode=indexing
        tunnel: [w1982] -> w1974 mode=indexing
        tunnel: w1975 -> [_]
        tunnel: [errorcluster {"status"=FALSE, "code"=0, "source"=""} ("error out")] -> w1976
        i -> [w1984]
        n957 = call "Beampointing get set motor position.vi"("Active CCD"=w1984, "get or set"=enum16{"get", "set"}."get", "dev variable alias Motors X"=w1987) -> ("Actual Position"=w1983:dbl)  [unwired: 7 in, 1 out]
        n958 = call "Beampointing get set motor position.vi"("Active CCD"=w1984, "get or set"=enum16{"get", "set"}."get", "dev variable alias Motors X"=w1988) -> ("Actual Position"=w1982:dbl)  [unwired: 7 in, 1 out]
      }
      n959 = Bundle By Name("Positions x"=w1973, "Positions y"=w1974) -> (w1980:cluster{})  [unwired: 1 out]
      n960 = call <userlib>:"Tick Count (ms)__ogtk.vi"("error in (no error)"=w1976) -> ("millisecond timer value"=w1977:u32)  [unwired: 9 in, 1 out]
      n961 = Subtract(x=w1977, y=w1979) -> (x-y=→"get pos time":u32)
    }
    frame Enabled {
    }
  }
  n962 = Unbundle By Name(w17) -> ("tdms ref"=w16:refnum<k34>)
  n963 = for {
    tunnel: w45 -> [w1991] mode=indexing
    tunnel: w44 -> [w1990]
    tunnel: [w1989] -> w15
    n964 = call "IMAQ Dispose"("Image"=w1991, "error in (no error)"=w1990) -> ("error out"=w1989:errorcluster)  [unwired: 4 in]
  }
  n965 = TDMS Close(8:w15, 11:w16) -> (0:→"error out 2":errorcluster)  [unwired: 1 out]
